vi "gen CE SEM Mask Table.vi"(6 "Mask Type Info":T2, 8 "error in (no error)":errorcluster, 9 "RU Type (0=Full Mask)":i32, 10 "Center Freq":dbl, 11 "SA Measurement in":refnum<class "SA Measurement.lvclass">) -> (0 "error out":errorcluster, 1 "SEM Lower Mask Table":T1(array[cluster]), 2 "SEM Upper Mask Table":T1(array[cluster]), 3 "SA Measurement out":refnum<class "SA Measurement.lvclass">)   [LabVIEW 2023, in "Spectrum Analyzer.lvlib" / "SA Measurement.lvclass"]
uses:
  SA Measurement.lvclass
  SA Measurement.lvclass/SA Measurement.ctl
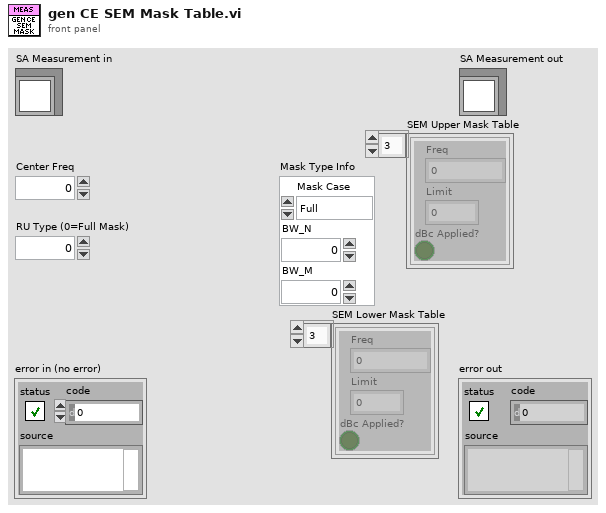
[diagram p1: front panel]
types:
  T1 = cluster{"Freq":dbl, "Limit":dbl, "dBc Applied?":bool}[]
  T2 = cluster{"Mask Case":enum16{"Full", "Case 1", "Case 2", "Case 3", "Case 1+2"}, "BW_N":dbl, "BW_M":dbl}
  T3 = cluster{"Freq":dbl, "Limit":dbl, "dBc Applied?":bool}
  T4 = enum16{"Full", "Case 1", "Case 2", "Case 3", "Case 1+2"}
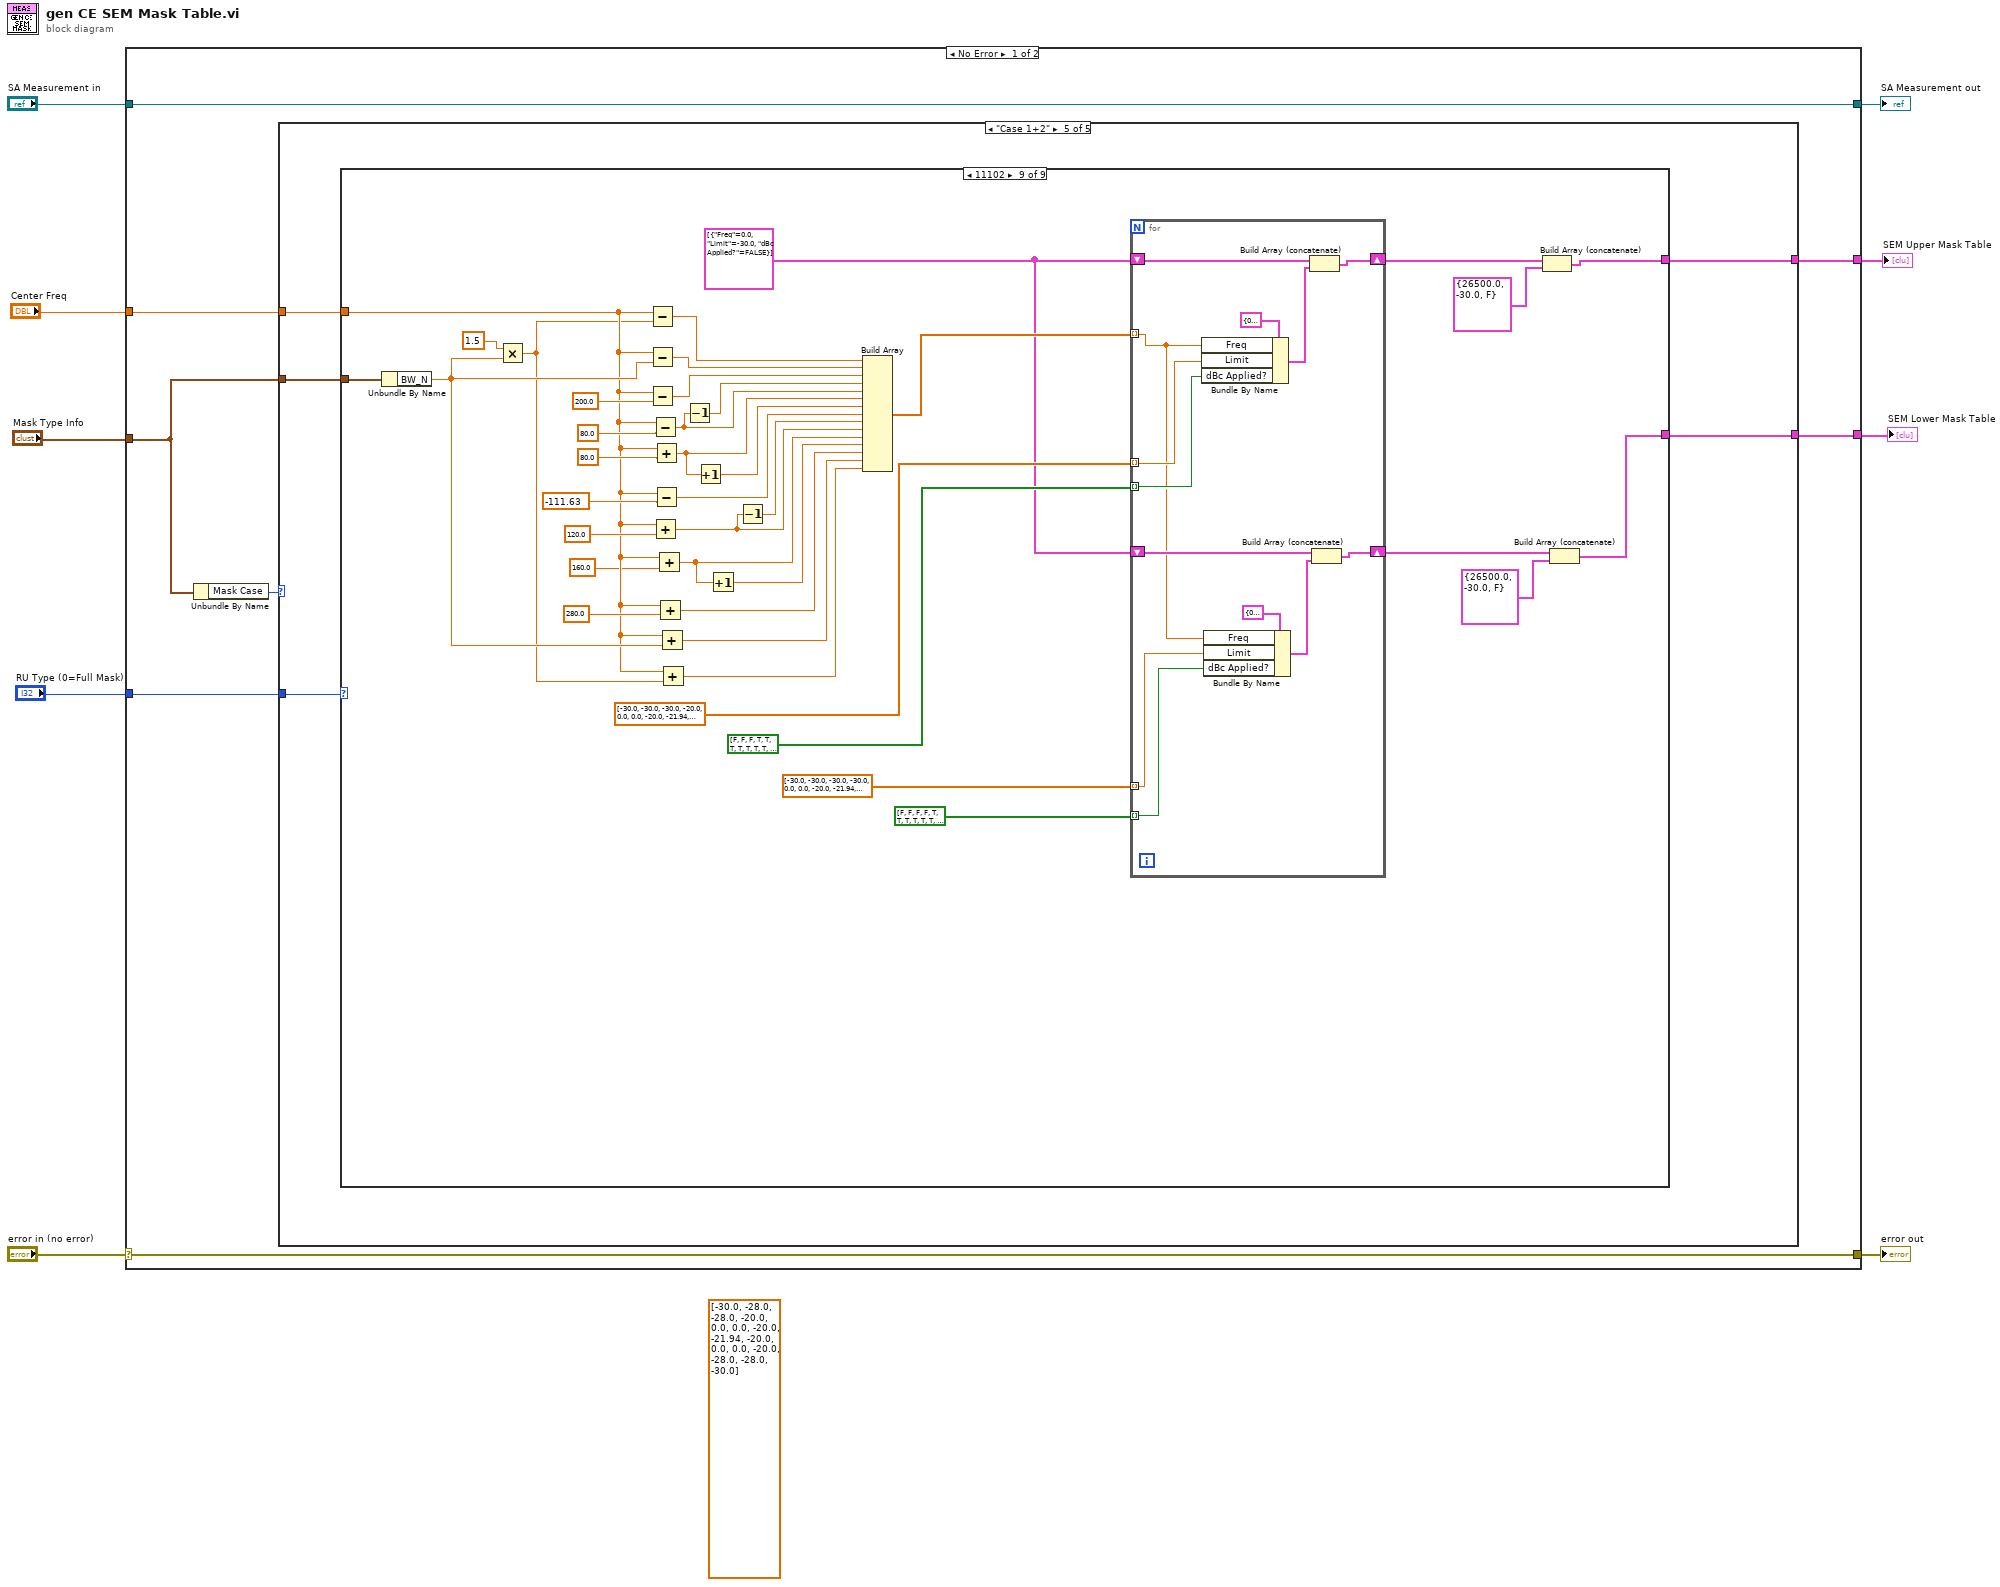
[diagram p0: block diagram]
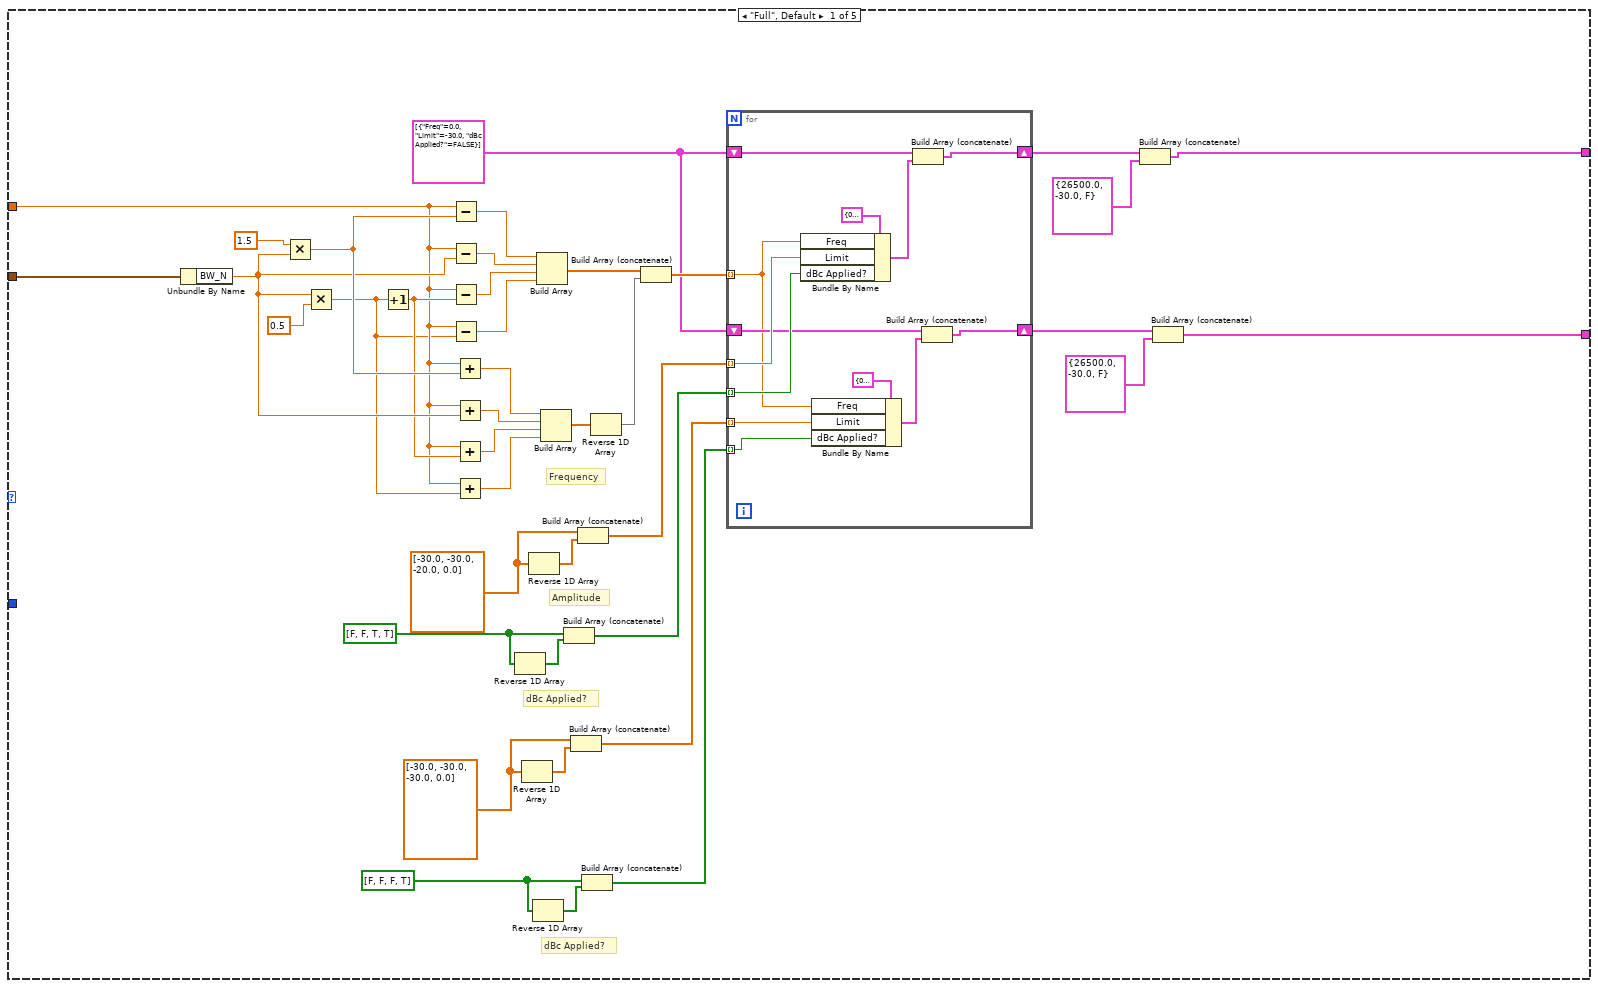
[diagram p2: hidden frame]
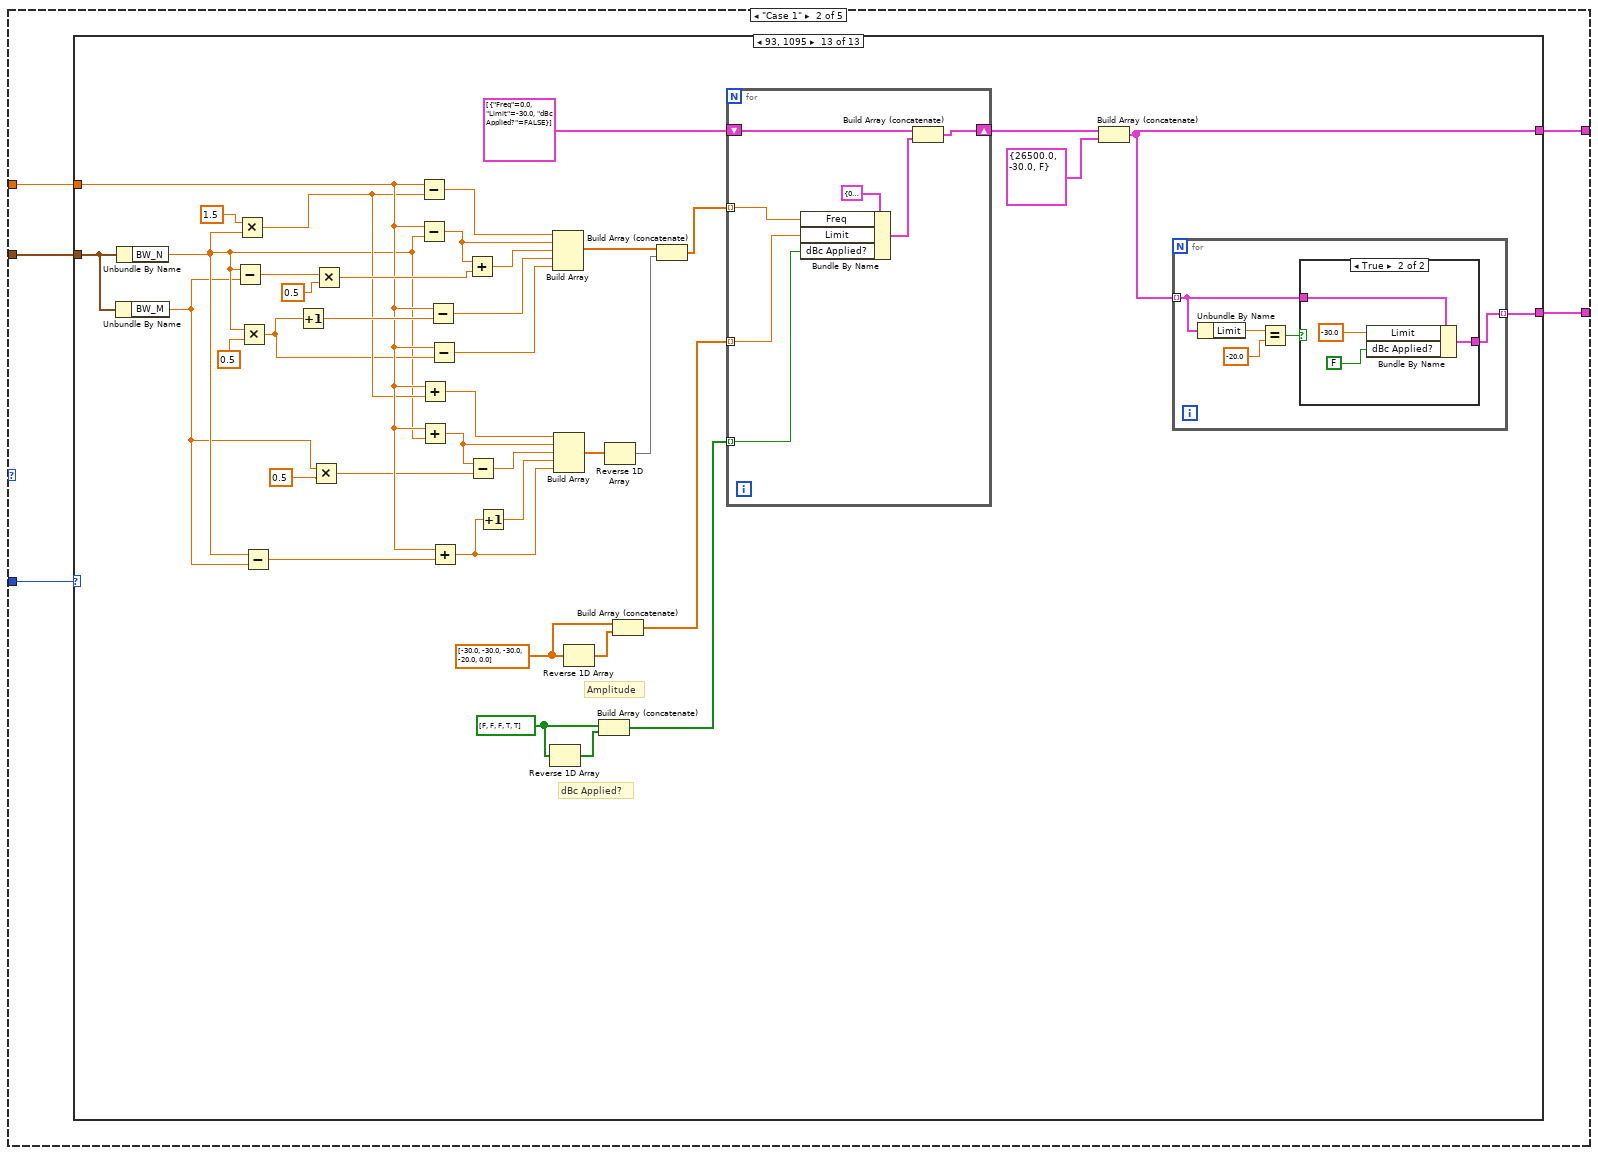
[diagram p3: hidden frame]
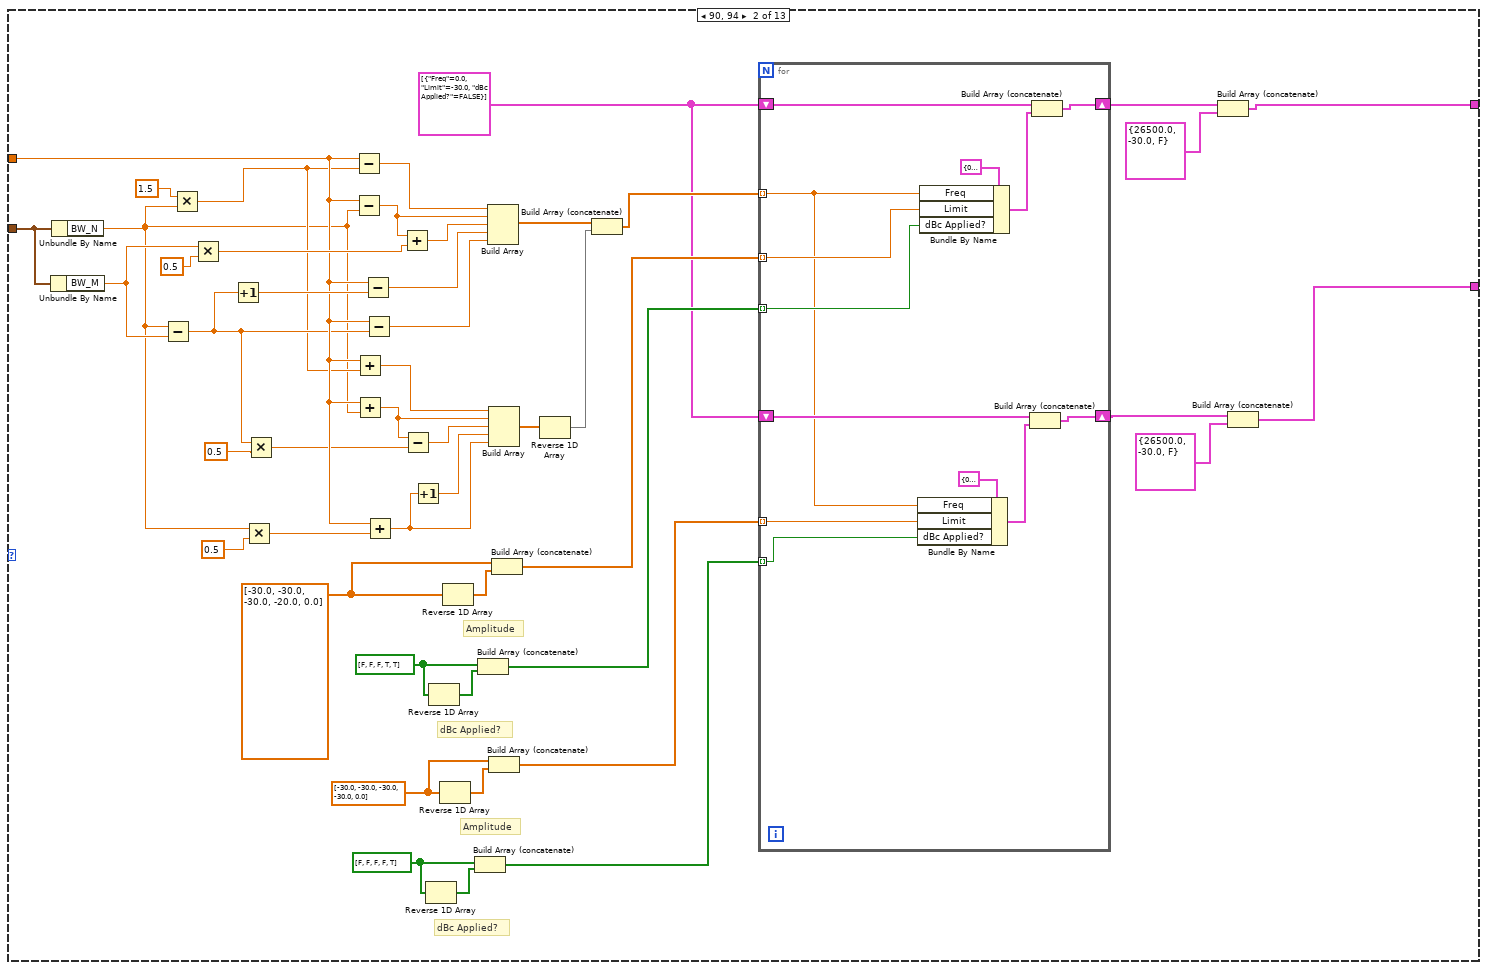
[diagram p5: hidden frame]
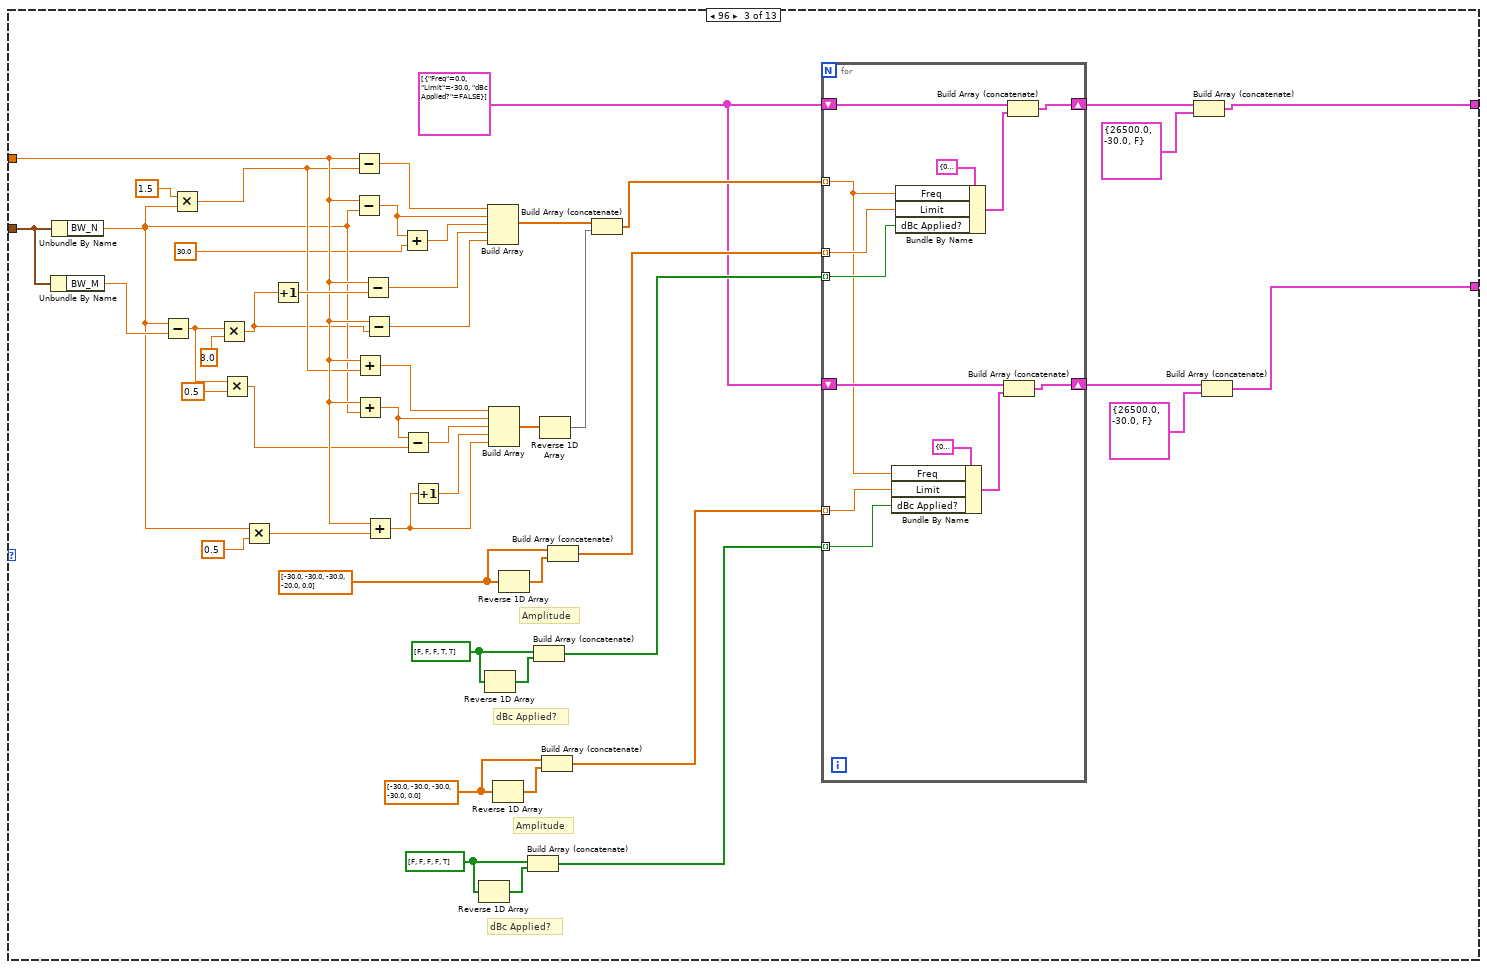
[diagram p6: hidden frame]
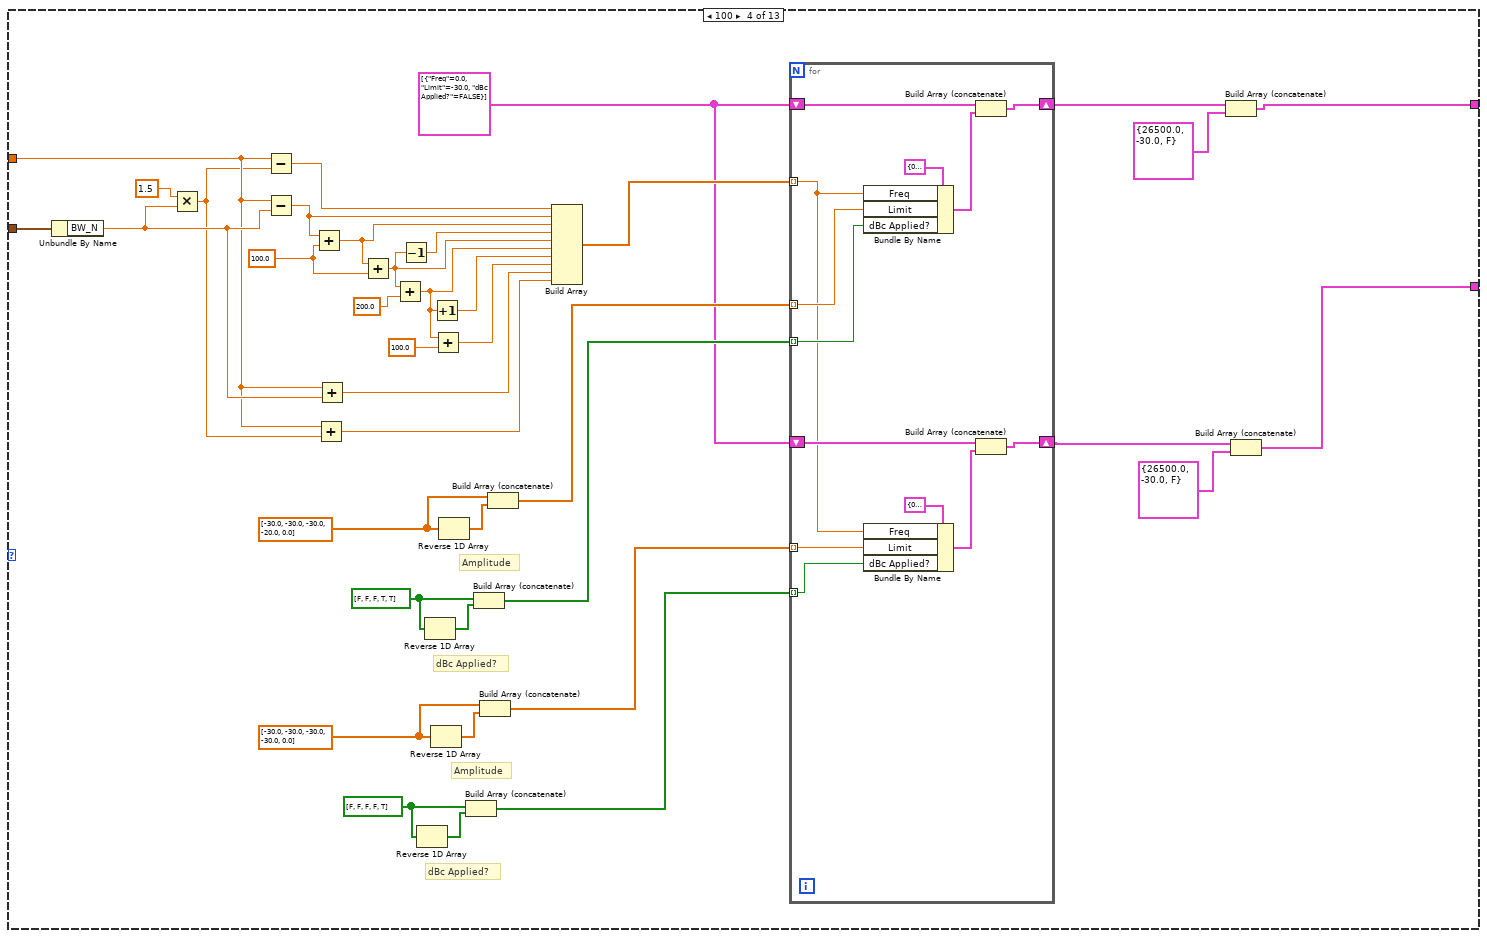
[diagram p7: hidden frame]
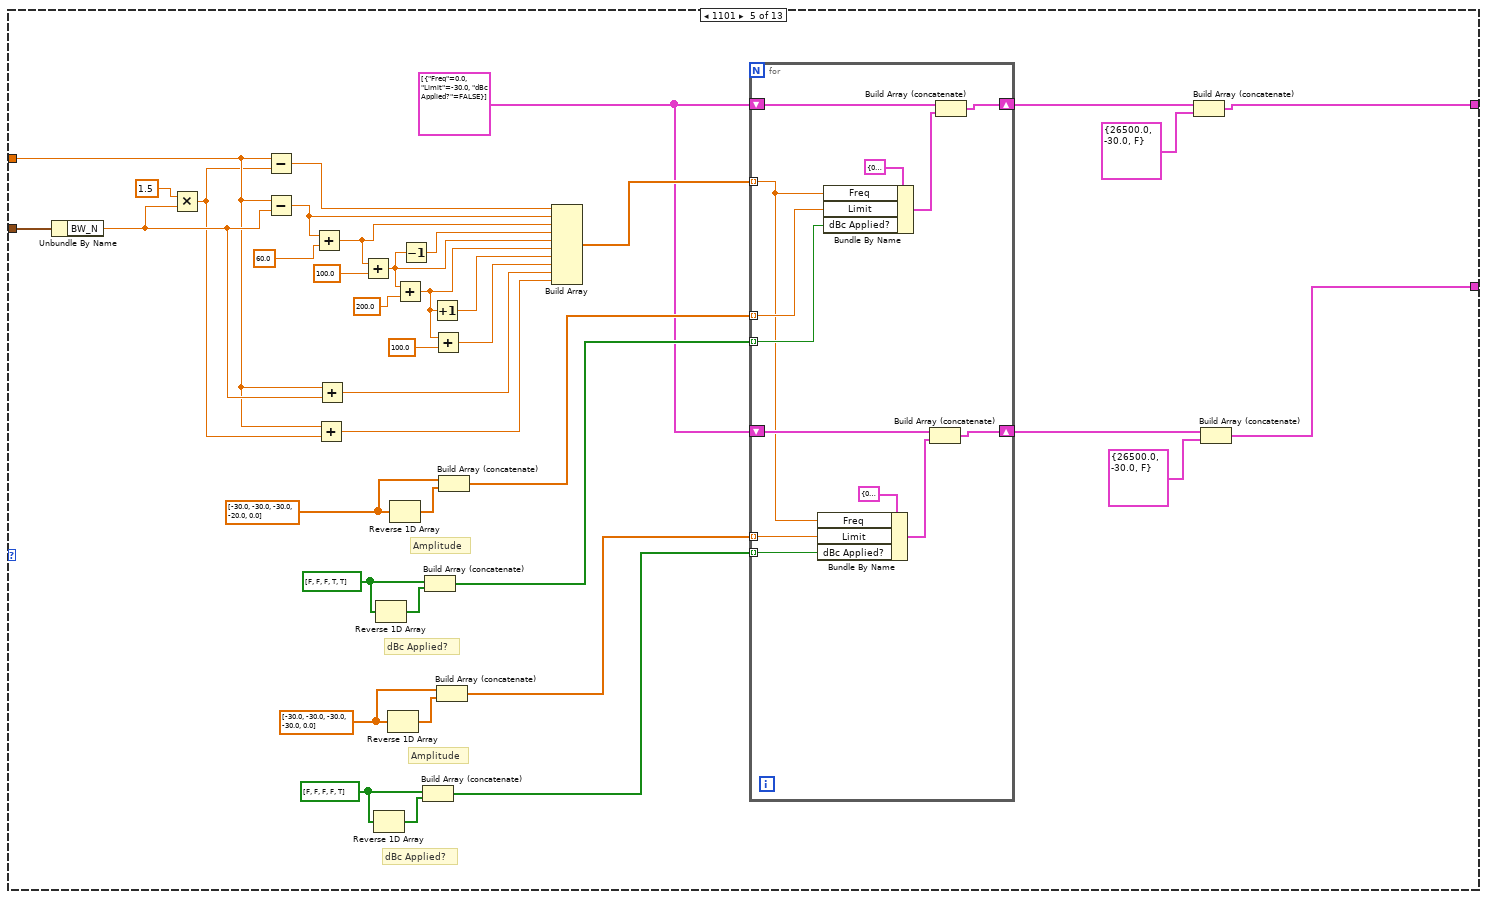
[diagram p8: hidden frame]
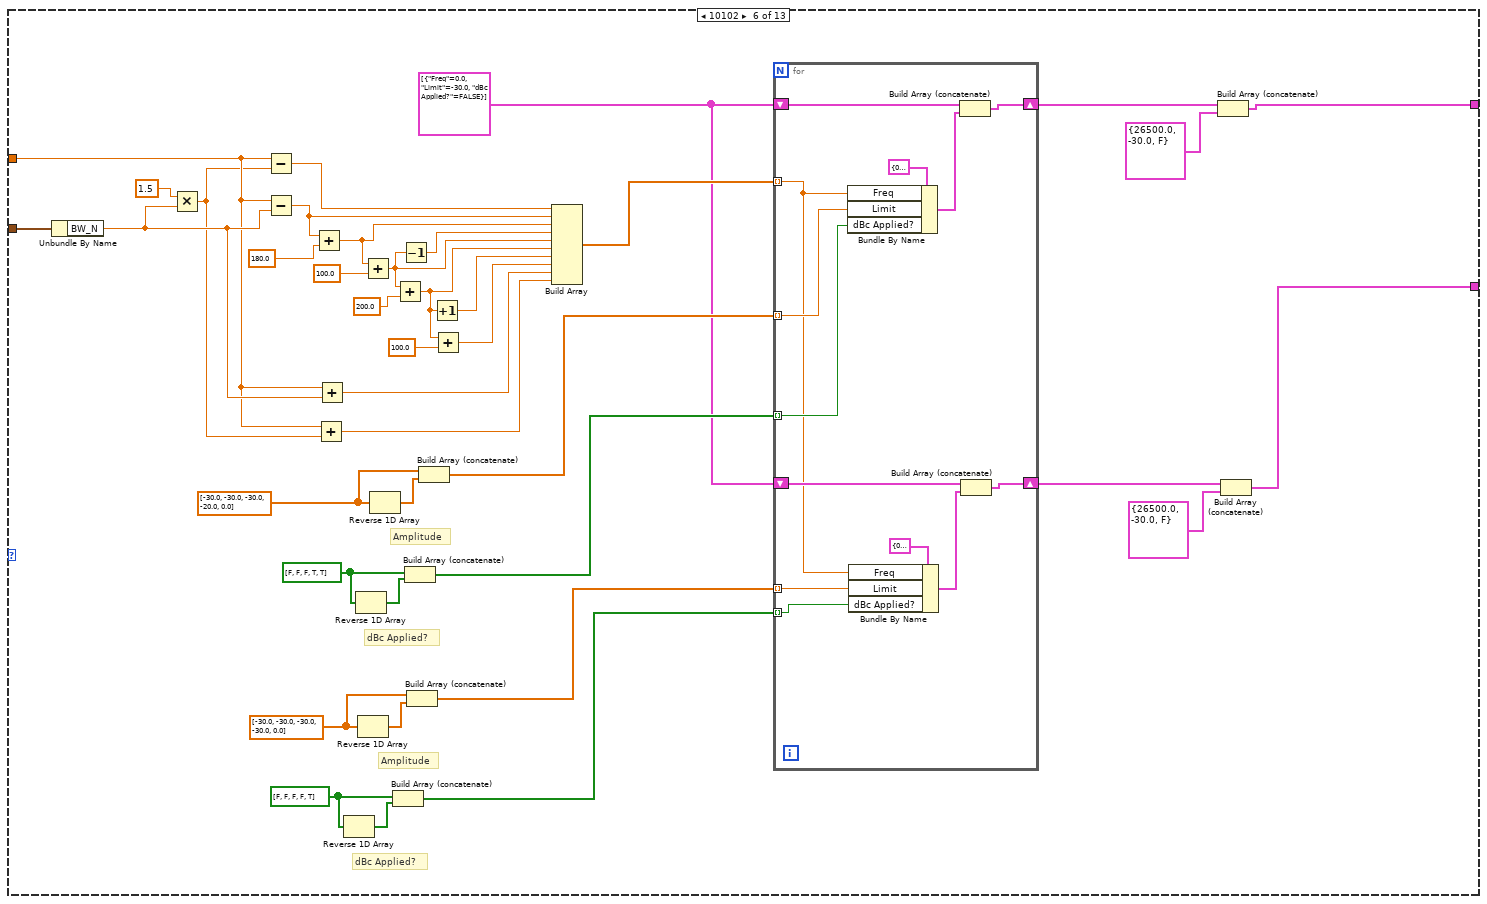
[diagram p9: hidden frame]
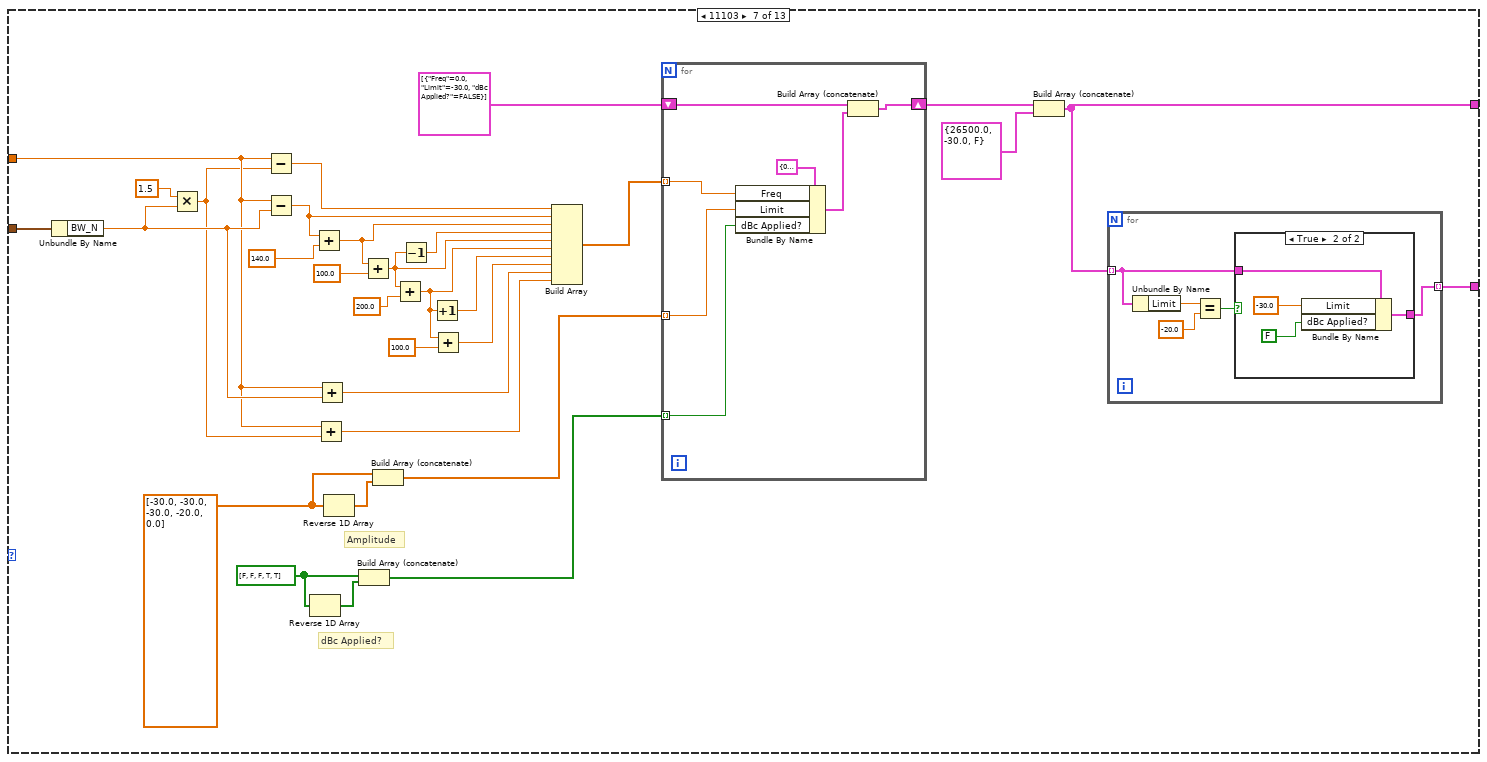
[diagram p10: hidden frame]
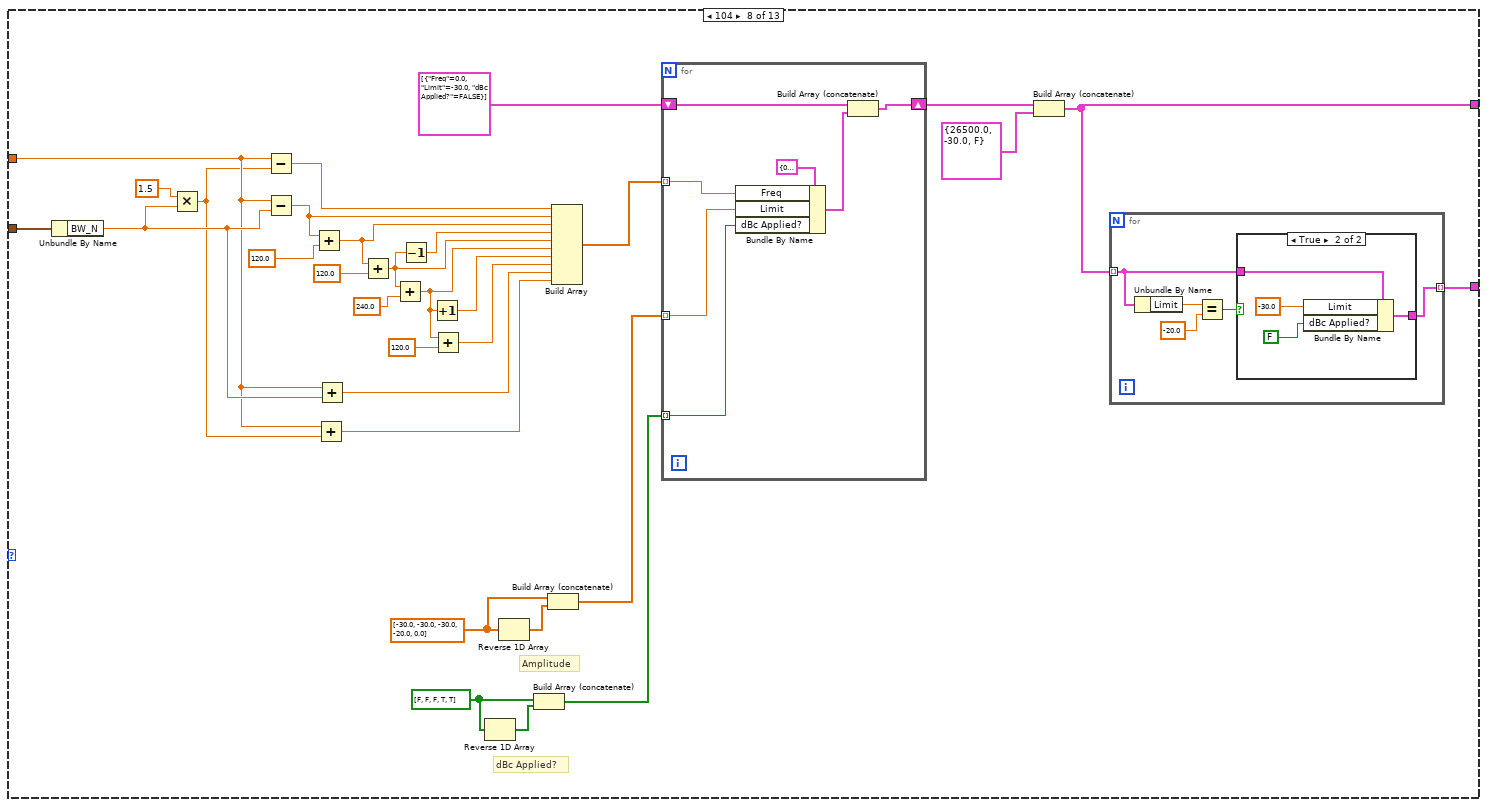
[diagram p12: hidden frame]
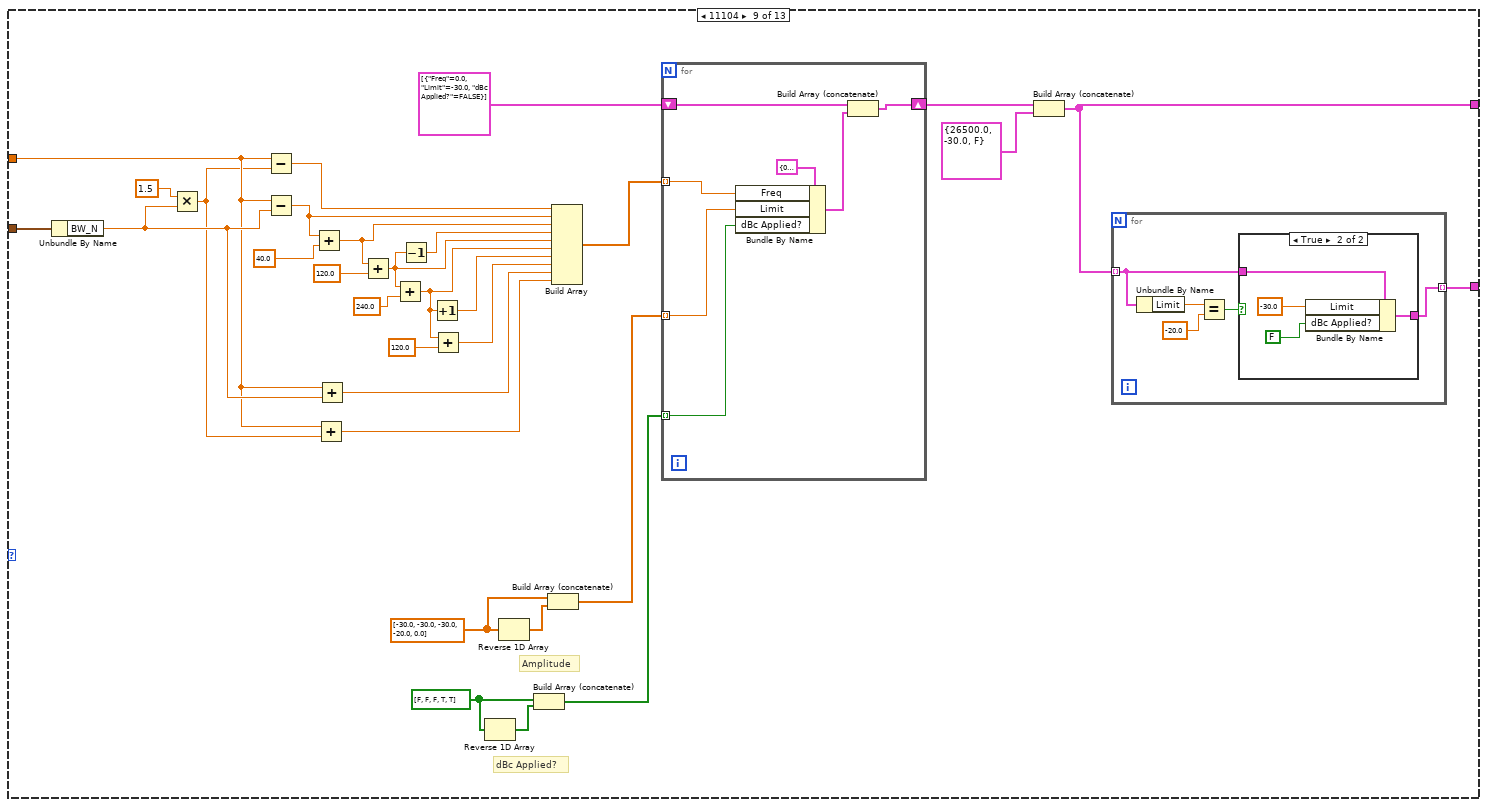
[diagram p14: hidden frame]
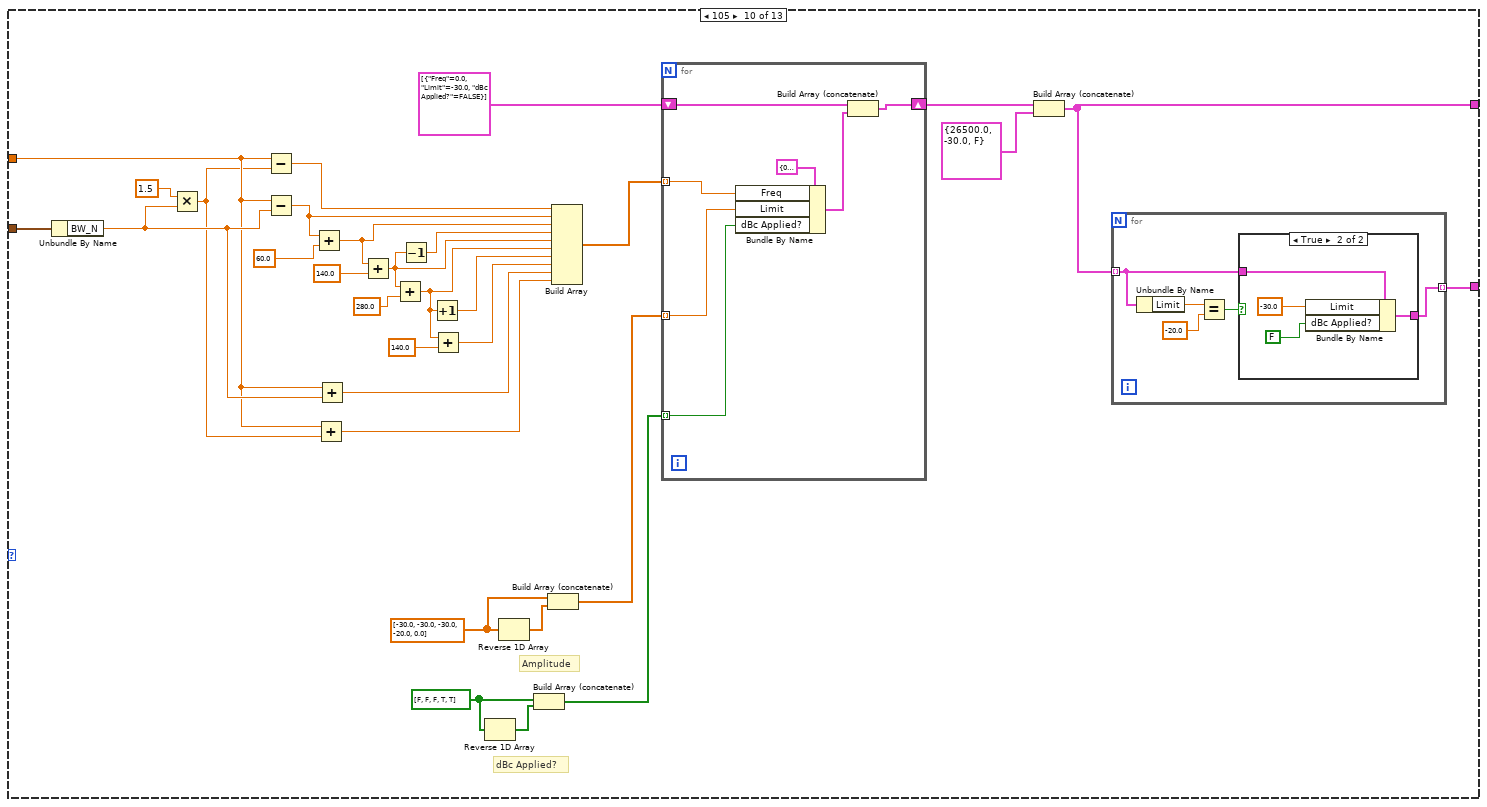
[diagram p16: hidden frame]
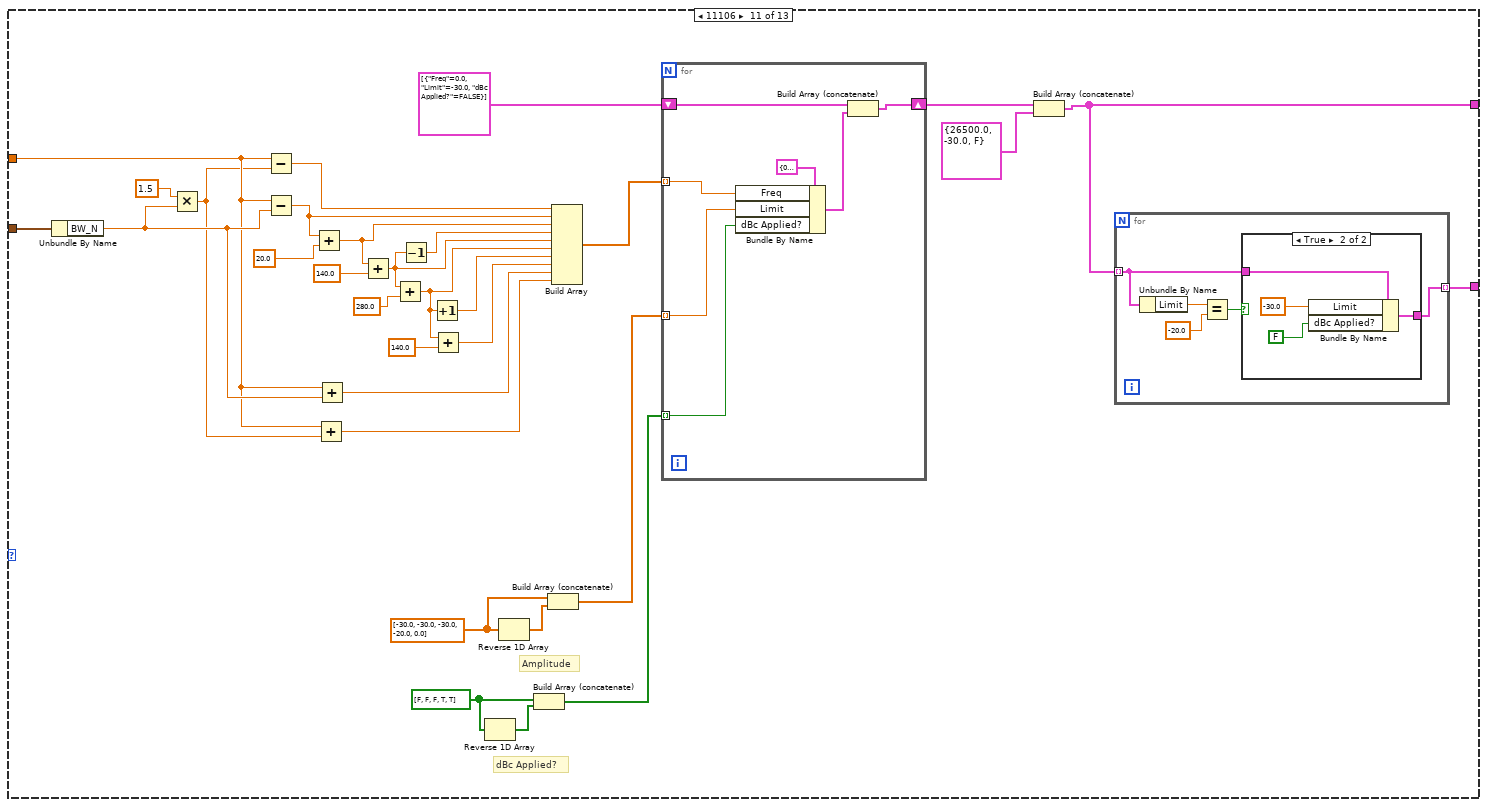
[diagram p18: hidden frame]
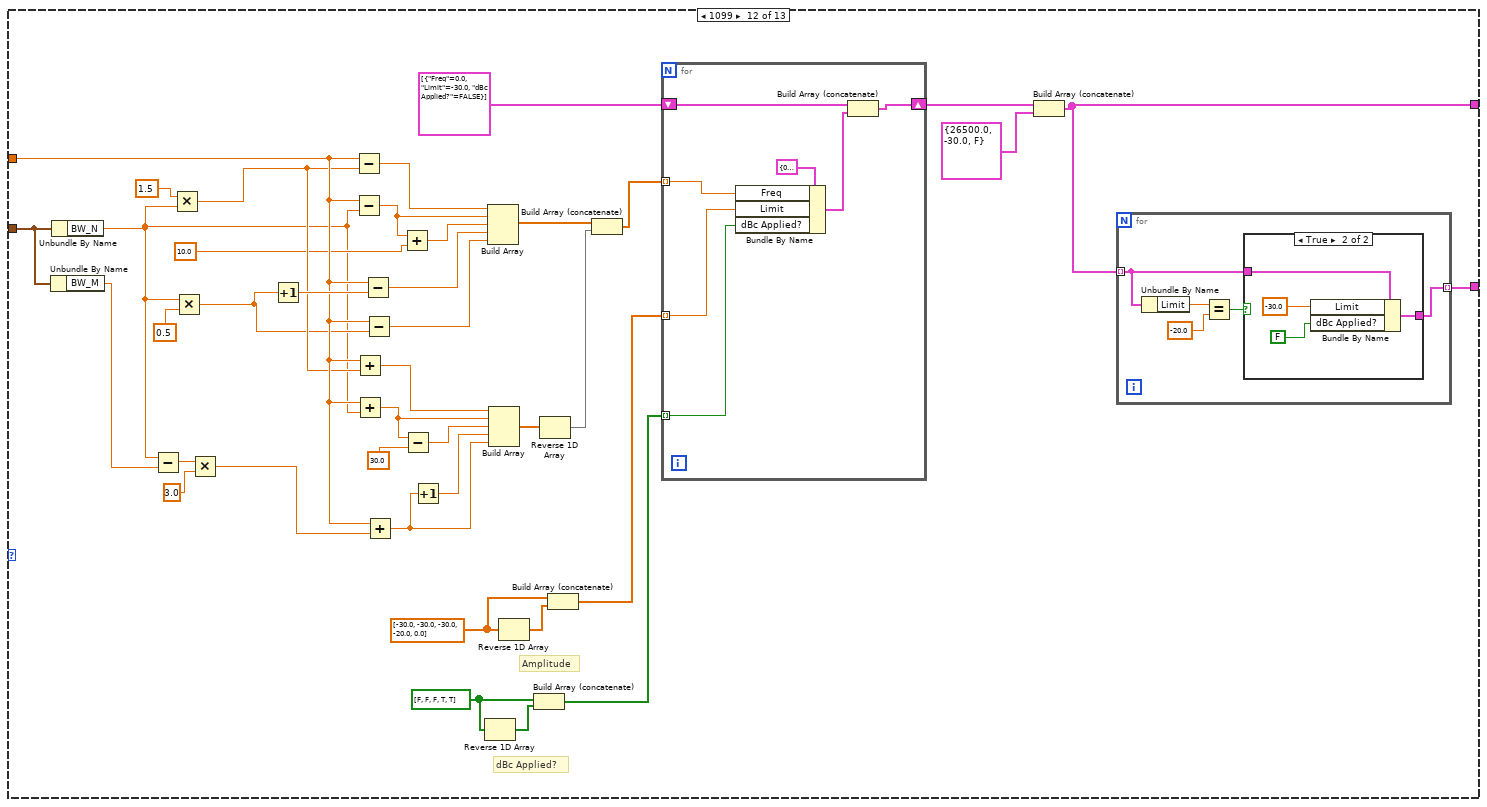
[diagram p20: hidden frame]
diagram:
  (unwired) dbl[] [-30.0, -28.0, -28.0, -20.0, 0.0, 0.0, -20.0, -21.94, -20.0, 0.0, 0.0, -20.0, -28.0, -28.0, -30.0]
  n1 = case shown="No Error" "error in (no error)" {
    selector: "error in (no error)" -> [w16 w2053]
    tunnel: [w16 w2053] -> w8
    tunnel: [w17 w2052] -> w6
    tunnel: "SA Measurement in" -> [w17 w2052]
    tunnel: "Mask Type Info" -> [w13 _]
    tunnel: "Center Freq" -> [w14 _]
    tunnel: "RU Type (0=Full Mask)" -> [w12 _]
    tunnel: [w11 _] -> w2
    tunnel: [w10 _] -> w1
    frame No Error {
      n2 = Unbundle By Name(w13) -> ("Mask Case"=w15:T4)
      n3 = case shown="\"Case 1+2\"" w15 {
        tunnel: w14 -> [w36 w72 w706 w1119 w1634]
        tunnel: w13 -> [w56 w73 w707 w1120 w1635]
        tunnel: [w28 w74 w708 w1121 w1636] -> w11
        tunnel: w12 -> [_ w71 w705 w1118 w1633]
        tunnel: [w24 w70 w704 w1117 w1632] -> w10
        frame "Full", Default {
          w20 = bool[] [FALSE, FALSE, FALSE, TRUE]
          w22 = dbl[] [-30.0, -30.0, -30.0, 0.0]
          w27 = T1 [{"Freq"=0.0, "Limit"=-30.0, "dBc Applied?"=FALSE}] ("value")
          w45 = bool[] [FALSE, FALSE, TRUE, TRUE]
          w49 = dbl[] [-30.0, -30.0, -20.0, 0.0]
          # "dBc Applied?"
          # "dBc Applied?"
          # "Amplitude"
          # "Frequency"
          n4 = Unbundle By Name(w56) -> ("BW_N"=w38:dbl)
          n5 = Multiply(x=1.5, y=w38) -> (x*y=w39:dbl)
          n6 = Multiply(x=w38, y=0.5) -> (x*y=w35:dbl)
          n7 = Increment(x=w35) -> (x+1=w37:dbl)
          n8 = Subtract(x=w36, y=w39) -> (x-y=w53:dbl)
          n9 = Subtract(x=w36, y=w38) -> (x-y=w52:dbl)
          n10 = Subtract(x=w36, y=w37) -> (x-y=w50:dbl)
          n11 = Subtract(x=w36, y=w35) -> (x-y=w51:dbl)
          n12 = Add(x=w36, y=w39) -> (x+y=w40:dbl)
          n13 = Add(x=w36, y=w38) -> (x+y=w41:dbl)
          n14 = Add(x=w36, y=w37) -> (x+y=w43:dbl)
          n15 = Add(x=w36, y=w35) -> (x+y=w42:dbl)
          n16 = Reverse 1D Array(array=w45) -> (reversed array=w46:bool[])
          n17 = Reverse 1D Array(array=w22) -> (reversed array=w23:dbl[])
          n18 = Reverse 1D Array(array=w49) -> (reversed array=w48:dbl[])
          n19 = Reverse 1D Array(array=w20) -> (reversed array=w19:bool[])
          n20 = Build Array(w53, w52, w50, w51) -> (w33:dbl[])
          n21 = Build Array(w40, w41, w43, w42) -> (w34:dbl[])
          n22 = Build Array (concatenate)(w45, w46) -> (w44:bool[])
          n23 = Build Array (concatenate)(w22, w23) -> (w21:dbl[])
          n24 = Build Array (concatenate)(w49, w48) -> (w47:dbl[])
          n25 = Build Array (concatenate)(w20, w19) -> (w18:bool[])
          n26 = Reverse 1D Array(array=w34) -> (reversed array=w32:dbl[])
          n27 = Build Array (concatenate)(w33, w32) -> (w31:dbl[])
          n28 = for {
            tunnel: w31 -> [w59] mode=indexing
            tunnel: w47 -> [w68] mode=indexing
            tunnel: w44 -> [w67] mode=indexing
            shift-right: [w64] -> w30
            shift-left: w27 -> [w66]
            shift-right: [w61] -> w25
            shift-left: w27 -> [w62]
            tunnel: w21 -> [w58] mode=indexing
            tunnel: w18 -> [w57] mode=indexing
            n29 = Bundle By Name(cluster=T3 {"Freq"=0.0, "Limit"=0.0, "dBc Applied?"=FALSE} ("Mask Table"), "Freq"=w59, "Limit"=w68, "dBc Applied?"=w67) -> (w65:T3)
            n30 = Bundle By Name(cluster=T3 {"Freq"=0.0, "Limit"=0.0, "dBc Applied?"=FALSE} ("Mask Table"), "Freq"=w59, "Limit"=w58, "dBc Applied?"=w57) -> (w60:T3)
            n31 = Build Array (concatenate)(w66, w65) -> (w64:T1)
            n32 = Build Array (concatenate)(w62, w60) -> (w61:T1)
          }
          n33 = Build Array (concatenate)(w30, T3 {"Freq"=26500.0, "Limit"=-30.0, "dBc Applied?"=FALSE} ("Mask Table")) -> (w28:T1)
          n34 = Build Array (concatenate)(w25, T3 {"Freq"=26500.0, "Limit"=-30.0, "dBc Applied?"=FALSE} ("Mask Table")) -> (w24:T1)
        }
        frame "Case 1" {
          n35 = case shown="93, 1095" w71 {
            tunnel: [_ w109 w171 w224 w276 w328 w352 w400 w448 w496 w544 w592 w648] -> w74
            tunnel: w73 -> [_ w108 w170 w223 w275 w327 w371 w419 w467 w515 w563 w617 w673]
            tunnel: w72 -> [_ w96 w159 w208 w260 w312 w356 w404 w452 w500 w548 w607 w662]
            tunnel: [_ w75 w135 w196 w247 w299 w351 w399 w447 w495 w543 w591 w647] -> w70
            frame 0, Default {
            }
            frame 90, 94 {
              w84 = dbl[] [-30.0, -30.0, -30.0, -30.0, 0.0]
              w83 = bool[] [FALSE, FALSE, FALSE, FALSE, TRUE]
              w106 = dbl[] [-30.0, -30.0, -30.0, -20.0, 0.0]
              w80 = T1 [{"Freq"=0.0, "Limit"=-30.0, "dBc Applied?"=FALSE}] ("value")
              w115 = bool[] [FALSE, FALSE, FALSE, TRUE, TRUE]
              # "dBc Applied?"
              # "Amplitude"
              # "dBc Applied?"
              # "Amplitude"
              n36 = Unbundle By Name(w108) -> ("BW_M"=w103:dbl)
              n37 = Unbundle By Name(w108) -> ("BW_N"=w91:dbl)
              n38 = Subtract(x=w91, y=w103) -> (x-y=w95:dbl)
              n39 = Multiply(x=1.5, y=w91) -> (x*y=w92:dbl)
              n40 = Multiply(x=w103, y=0.5) -> (x*y=w104:dbl)
              n41 = Increment(x=w95) -> (x+1=w102:dbl)
              n42 = Multiply(x=w91, y=0.5) -> (x*y=w89:dbl)
              n43 = Multiply(x=w95, y=0.5) -> (x*y=w93:dbl)
              n44 = Subtract(x=w96, y=w92) -> (x-y=w119:dbl)
              n45 = Subtract(x=w96, y=w91) -> (x-y=w105:dbl)
              n46 = Add(x=w96, y=w92) -> (x+y=w97:dbl)
              n47 = Add(x=w96, y=w91) -> (x+y=w99:dbl)
              n48 = Subtract(x=w96, y=w102) -> (x-y=w101:dbl)
              n49 = Subtract(x=w96, y=w95) -> (x-y=w100:dbl)
              n50 = Add(x=w96, y=w89) -> (x+y=w88:dbl)
              n51 = Add(x=w105, y=w104) -> (x+y=w107:dbl)
              n52 = Subtract(x=w99, y=w93) -> (x-y=w98:dbl)
              n53 = Increment(x=w88) -> (x+1=w87:dbl)
              n54 = Reverse 1D Array(array=w83) -> (reversed array=w82:bool[])
              n55 = Reverse 1D Array(array=w115) -> (reversed array=w116:bool[])
              n56 = Reverse 1D Array(array=w84) -> (reversed array=w81:dbl[])
              n57 = Reverse 1D Array(array=w106) -> (reversed array=w118:dbl[])
              n58 = Build Array (concatenate)(w83, w82) -> (w78:bool[])
              n59 = Build Array (concatenate)(w115, w116) -> (w114:bool[])
              n60 = Build Array(w119, w105, w107, w101, w100) -> (w113:dbl[])
              n61 = Build Array(w97, w99, w98, w87, w88) -> (w86:dbl[])
              n62 = Build Array (concatenate)(w84, w81) -> (w79:dbl[])
              n63 = Build Array (concatenate)(w106, w118) -> (w117:dbl[])
              n64 = Reverse 1D Array(array=w86) -> (reversed array=w85:dbl[])
              n65 = Build Array (concatenate)(w113, w85) -> (w112:dbl[])
              n66 = for {
                tunnel: w112 -> [w124] mode=indexing
                tunnel: w117 -> [w133] mode=indexing
                tunnel: w114 -> [w132] mode=indexing
                shift-right: [w129] -> w111
                shift-left: w80 -> [w131]
                shift-right: [w125] -> w76
                shift-left: w80 -> [w126]
                tunnel: w79 -> [w123] mode=indexing
                tunnel: w78 -> [w122] mode=indexing
                n67 = Bundle By Name(cluster=T3 {"Freq"=0.0, "Limit"=0.0, "dBc Applied?"=FALSE} ("Mask Table"), "Freq"=w124, "Limit"=w123, "dBc Applied?"=w122) -> (w128:T3)
                n68 = Bundle By Name(cluster=T3 {"Freq"=0.0, "Limit"=0.0, "dBc Applied?"=FALSE} ("Mask Table"), "Freq"=w124, "Limit"=w133, "dBc Applied?"=w132) -> (w130:T3)
                n69 = Build Array (concatenate)(w126, w128) -> (w125:T1)
                n70 = Build Array (concatenate)(w131, w130) -> (w129:T1)
              }
              n71 = Build Array (concatenate)(w111, T3 {"Freq"=26500.0, "Limit"=-30.0, "dBc Applied?"=FALSE} ("Mask Table")) -> (w109:T1)
              n72 = Build Array (concatenate)(w76, T3 {"Freq"=26500.0, "Limit"=-30.0, "dBc Applied?"=FALSE} ("Mask Table")) -> (w75:T1)
            }
            frame 96 {
              w144 = dbl[] [-30.0, -30.0, -30.0, -30.0, 0.0]
              w143 = bool[] [FALSE, FALSE, FALSE, FALSE, TRUE]
              w168 = dbl[] [-30.0, -30.0, -30.0, -20.0, 0.0]
              w139 = T1 [{"Freq"=0.0, "Limit"=-30.0, "dBc Applied?"=FALSE}] ("value")
              w177 = bool[] [FALSE, FALSE, FALSE, TRUE, TRUE]
              # "dBc Applied?"
              # "Amplitude"
              # "dBc Applied?"
              # "Amplitude"
              n73 = Unbundle By Name(w170) -> ("BW_M"=w166:dbl)
              n74 = Unbundle By Name(w170) -> ("BW_N"=w157:dbl)
              n75 = Subtract(x=w157, y=w166) -> (x-y=w148:dbl)
              n76 = Multiply(x=1.5, y=w157) -> (x*y=w158:dbl)
              n77 = Multiply(x=w148, y=3.0) -> (x*y=w146:dbl)
              n78 = Multiply(x=w148, y=0.5) -> (x*y=w145:dbl)
              n79 = Multiply(x=w157, y=0.5) -> (x*y=w155:dbl)
              n80 = Increment(x=w146) -> (x+1=w165:dbl)
              n81 = Subtract(x=w159, y=w158) -> (x-y=w181:dbl)
              n82 = Subtract(x=w159, y=w157) -> (x-y=w167:dbl)
              n83 = Add(x=w159, y=w158) -> (x+y=w160:dbl)
              n84 = Add(x=w159, y=w157) -> (x+y=w162:dbl)
              n85 = Subtract(x=w159, y=w165) -> (x-y=w164:dbl)
              n86 = Subtract(x=w159, y=w146) -> (x-y=w163:dbl)
              n87 = Add(x=w159, y=w155) -> (x+y=w154:dbl)
              n88 = Add(x=w167, y=30.0 ("x")) -> (x+y=w169:dbl)
              n89 = Subtract(x=w162, y=w145) -> (x-y=w161:dbl)
              n90 = Increment(x=w154) -> (x+1=w153:dbl)
              n91 = Reverse 1D Array(array=w143) -> (reversed array=w142:bool[])
              n92 = Reverse 1D Array(array=w177) -> (reversed array=w178:bool[])
              n93 = Build Array(w181, w167, w169, w164, w163) -> (w175:dbl[])
              n94 = Build Array(w160, w162, w161, w153, w154) -> (w152:dbl[])
              n95 = Reverse 1D Array(array=w144) -> (reversed array=w141:dbl[])
              n96 = Reverse 1D Array(array=w168) -> (reversed array=w180:dbl[])
              n97 = Build Array (concatenate)(w143, w142) -> (w138:bool[])
              n98 = Build Array (concatenate)(w177, w178) -> (w176:bool[])
              n99 = Reverse 1D Array(array=w152) -> (reversed array=w151:dbl[])
              n100 = Build Array (concatenate)(w144, w141) -> (w140:dbl[])
              n101 = Build Array (concatenate)(w168, w180) -> (w179:dbl[])
              n102 = Build Array (concatenate)(w175, w151) -> (w174:dbl[])
              n103 = for {
                tunnel: w174 -> [w185] mode=indexing
                tunnel: w179 -> [w194] mode=indexing
                tunnel: w176 -> [w193] mode=indexing
                shift-right: [w190] -> w173
                shift-left: w139 -> [w192]
                tunnel: w140 -> [w184] mode=indexing
                shift-right: [w186] -> w136
                shift-left: w139 -> [w187]
                tunnel: w138 -> [w183] mode=indexing
                n104 = Bundle By Name(cluster=T3 {"Freq"=0.0, "Limit"=0.0, "dBc Applied?"=FALSE} ("Mask Table"), "Freq"=w185, "Limit"=w184, "dBc Applied?"=w183) -> (w189:T3)
                n105 = Bundle By Name(cluster=T3 {"Freq"=0.0, "Limit"=0.0, "dBc Applied?"=FALSE} ("Mask Table"), "Freq"=w185, "Limit"=w194, "dBc Applied?"=w193) -> (w191:T3)
                n106 = Build Array (concatenate)(w187, w189) -> (w186:T1)
                n107 = Build Array (concatenate)(w192, w191) -> (w190:T1)
              }
              n108 = Build Array (concatenate)(w173, T3 {"Freq"=26500.0, "Limit"=-30.0, "dBc Applied?"=FALSE} ("Mask Table")) -> (w171:T1)
              n109 = Build Array (concatenate)(w136, T3 {"Freq"=26500.0, "Limit"=-30.0, "dBc Applied?"=FALSE} ("Mask Table")) -> (w135:T1)
            }
            frame 100 {
              w204 = dbl[] [-30.0, -30.0, -30.0, -30.0, 0.0]
              w203 = bool[] [FALSE, FALSE, FALSE, FALSE, TRUE]
              w219 = 100.0 ("x")
              w222 = dbl[] [-30.0, -30.0, -30.0, -20.0, 0.0]
              w205 = T1 [{"Freq"=0.0, "Limit"=-30.0, "dBc Applied?"=FALSE}] ("value")
              w228 = bool[] [FALSE, FALSE, FALSE, TRUE, TRUE]
              # "dBc Applied?"
              # "Amplitude"
              # "dBc Applied?"
              # "Amplitude"
              n110 = Unbundle By Name(w223) -> ("BW_N"=w210:dbl)
              n111 = Multiply(x=1.5, y=w210) -> (x*y=w207:dbl)
              n112 = Subtract(x=w208, y=w207) -> (x-y=w232:dbl)
              n113 = Subtract(x=w208, y=w210) -> (x-y=w221:dbl)
              n114 = Add(x=w221, y=w219) -> (x+y=w220:dbl)
              n115 = Add(x=w208, y=w207) -> (x+y=w206:dbl)
              n116 = Add(x=w208, y=w210) -> (x+y=w209:dbl)
              n117 = Add(x=w220, y=w219) -> (x+y=w216:dbl)
              n118 = Add(x=w216, y=200.0) -> (x+y=w213:dbl)
              n119 = Decrement(x=w216) -> (x-1=w218:dbl)
              n120 = Reverse 1D Array(array=w203) -> (reversed array=w202:bool[])
              n121 = Reverse 1D Array(array=w228) -> (reversed array=w229:bool[])
              n122 = Reverse 1D Array(array=w204) -> (reversed array=w201:dbl[])
              n123 = Increment(x=w213) -> (x+1=w214:dbl)
              n124 = Add(x=w213, y=100.0) -> (x+y=w211:dbl)
              n125 = Reverse 1D Array(array=w222) -> (reversed array=w231:dbl[])
              n126 = Build Array (concatenate)(w203, w202) -> (w199:bool[])
              n127 = Build Array (concatenate)(w228, w229) -> (w227:bool[])
              n128 = Build Array (concatenate)(w204, w201) -> (w200:dbl[])
              n129 = Build Array (concatenate)(w222, w231) -> (w230:dbl[])
              n130 = Build Array(w232, w221, w220, w218, w216, w213, w214, w211, w209, w206) -> (w217:dbl[])
              n131 = for {
                tunnel: w217 -> [w236] mode=indexing
                tunnel: w230 -> [w245] mode=indexing
                tunnel: w227 -> [w244] mode=indexing
                shift-right: [w241] -> w226
                shift-left: w205 -> [w243]
                shift-right: [w237] -> w197
                shift-left: w205 -> [w238]
                tunnel: w200 -> [w235] mode=indexing
                tunnel: w199 -> [w234] mode=indexing
                n132 = Bundle By Name(cluster=T3 {"Freq"=0.0, "Limit"=0.0, "dBc Applied?"=FALSE} ("Mask Table"), "Freq"=w236, "Limit"=w245, "dBc Applied?"=w244) -> (w242:T3)
                n133 = Bundle By Name(cluster=T3 {"Freq"=0.0, "Limit"=0.0, "dBc Applied?"=FALSE} ("Mask Table"), "Freq"=w236, "Limit"=w235, "dBc Applied?"=w234) -> (w240:T3)
                n134 = Build Array (concatenate)(w243, w242) -> (w241:T1)
                n135 = Build Array (concatenate)(w238, w240) -> (w237:T1)
              }
              n136 = Build Array (concatenate)(w226, T3 {"Freq"=26500.0, "Limit"=-30.0, "dBc Applied?"=FALSE} ("Mask Table")) -> (w224:T1)
              n137 = Build Array (concatenate)(w197, T3 {"Freq"=26500.0, "Limit"=-30.0, "dBc Applied?"=FALSE} ("Mask Table")) -> (w196:T1)
            }
            frame 1101 {
              w255 = dbl[] [-30.0, -30.0, -30.0, -30.0, 0.0]
              w254 = bool[] [FALSE, FALSE, FALSE, FALSE, TRUE]
              w274 = dbl[] [-30.0, -30.0, -30.0, -20.0, 0.0]
              w256 = T1 [{"Freq"=0.0, "Limit"=-30.0, "dBc Applied?"=FALSE}] ("value")
              w280 = bool[] [FALSE, FALSE, FALSE, TRUE, TRUE]
              # "dBc Applied?"
              # "Amplitude"
              # "dBc Applied?"
              # "Amplitude"
              n138 = Unbundle By Name(w275) -> ("BW_N"=w262:dbl)
              n139 = Multiply(x=1.5, y=w262) -> (x*y=w259:dbl)
              n140 = Subtract(x=w260, y=w259) -> (x-y=w284:dbl)
              n141 = Subtract(x=w260, y=w262) -> (x-y=w273:dbl)
              n142 = Add(x=w273, y=60.0 ("x")) -> (x+y=w272:dbl)
              n143 = Add(x=w260, y=w259) -> (x+y=w258:dbl)
              n144 = Add(x=w260, y=w262) -> (x+y=w261:dbl)
              n145 = Add(x=w272, y=100.0) -> (x+y=w268:dbl)
              n146 = Reverse 1D Array(array=w254) -> (reversed array=w253:bool[])
              n147 = Reverse 1D Array(array=w280) -> (reversed array=w281:bool[])
              n148 = Reverse 1D Array(array=w255) -> (reversed array=w252:dbl[])
              n149 = Reverse 1D Array(array=w274) -> (reversed array=w283:dbl[])
              n150 = Add(x=w268, y=200.0) -> (x+y=w265:dbl)
              n151 = Decrement(x=w268) -> (x-1=w270:dbl)
              n152 = Build Array (concatenate)(w254, w253) -> (w250:bool[])
              n153 = Build Array (concatenate)(w280, w281) -> (w279:bool[])
              n154 = Increment(x=w265) -> (x+1=w266:dbl)
              n155 = Add(x=w265, y=100.0) -> (x+y=w263:dbl)
              n156 = Build Array (concatenate)(w255, w252) -> (w251:dbl[])
              n157 = Build Array (concatenate)(w274, w283) -> (w282:dbl[])
              n158 = Build Array(w284, w273, w272, w270, w268, w265, w266, w263, w261, w258) -> (w269:dbl[])
              n159 = for {
                tunnel: w269 -> [w288] mode=indexing
                tunnel: w282 -> [w297] mode=indexing
                tunnel: w279 -> [w296] mode=indexing
                shift-right: [w293] -> w278
                shift-left: w256 -> [w295]
                shift-right: [w289] -> w248
                shift-left: w256 -> [w290]
                tunnel: w251 -> [w287] mode=indexing
                tunnel: w250 -> [w286] mode=indexing
                n160 = Bundle By Name(cluster=T3 {"Freq"=0.0, "Limit"=0.0, "dBc Applied?"=FALSE} ("Mask Table"), "Freq"=w288, "Limit"=w287, "dBc Applied?"=w286) -> (w292:T3)
                n161 = Bundle By Name(cluster=T3 {"Freq"=0.0, "Limit"=0.0, "dBc Applied?"=FALSE} ("Mask Table"), "Freq"=w288, "Limit"=w297, "dBc Applied?"=w296) -> (w294:T3)
                n162 = Build Array (concatenate)(w290, w292) -> (w289:T1)
                n163 = Build Array (concatenate)(w295, w294) -> (w293:T1)
              }
              n164 = Build Array (concatenate)(w278, T3 {"Freq"=26500.0, "Limit"=-30.0, "dBc Applied?"=FALSE} ("Mask Table")) -> (w276:T1)
              n165 = Build Array (concatenate)(w248, T3 {"Freq"=26500.0, "Limit"=-30.0, "dBc Applied?"=FALSE} ("Mask Table")) -> (w247:T1)
            }
            frame 10102 {
              w307 = dbl[] [-30.0, -30.0, -30.0, -30.0, 0.0]
              w306 = bool[] [FALSE, FALSE, FALSE, FALSE, TRUE]
              w326 = dbl[] [-30.0, -30.0, -30.0, -20.0, 0.0]
              w308 = T1 [{"Freq"=0.0, "Limit"=-30.0, "dBc Applied?"=FALSE}] ("value")
              w332 = bool[] [FALSE, FALSE, FALSE, TRUE, TRUE]
              # "dBc Applied?"
              # "Amplitude"
              # "dBc Applied?"
              # "Amplitude"
              n166 = Unbundle By Name(w327) -> ("BW_N"=w314:dbl)
              n167 = Multiply(x=1.5, y=w314) -> (x*y=w311:dbl)
              n168 = Subtract(x=w312, y=w311) -> (x-y=w336:dbl)
              n169 = Subtract(x=w312, y=w314) -> (x-y=w325:dbl)
              n170 = Add(x=w325, y=180.0 ("x")) -> (x+y=w324:dbl)
              n171 = Add(x=w312, y=w311) -> (x+y=w310:dbl)
              n172 = Add(x=w312, y=w314) -> (x+y=w313:dbl)
              n173 = Reverse 1D Array(array=w306) -> (reversed array=w305:bool[])
              n174 = Reverse 1D Array(array=w332) -> (reversed array=w333:bool[])
              n175 = Reverse 1D Array(array=w307) -> (reversed array=w304:dbl[])
              n176 = Add(x=w324, y=100.0) -> (x+y=w320:dbl)
              n177 = Reverse 1D Array(array=w326) -> (reversed array=w335:dbl[])
              n178 = Build Array (concatenate)(w306, w305) -> (w302:bool[])
              n179 = Add(x=w320, y=200.0) -> (x+y=w317:dbl)
              n180 = Decrement(x=w320) -> (x-1=w322:dbl)
              n181 = Build Array (concatenate)(w332, w333) -> (w331:bool[])
              n182 = Build Array (concatenate)(w307, w304) -> (w303:dbl[])
              n183 = Build Array (concatenate)(w326, w335) -> (w334:dbl[])
              n184 = Increment(x=w317) -> (x+1=w318:dbl)
              n185 = Add(x=w317, y=100.0) -> (x+y=w315:dbl)
              n186 = Build Array(w336, w325, w324, w322, w320, w317, w318, w315, w313, w310) -> (w321:dbl[])
              n187 = for {
                tunnel: w321 -> [w340] mode=indexing
                tunnel: w334 -> [w349] mode=indexing
                tunnel: w331 -> [w348] mode=indexing
                shift-right: [w345] -> w330
                shift-left: w308 -> [w347]
                shift-right: [w341] -> w300
                shift-left: w308 -> [w342]
                tunnel: w303 -> [w339] mode=indexing
                tunnel: w302 -> [w338] mode=indexing
                n188 = Bundle By Name(cluster=T3 {"Freq"=0.0, "Limit"=0.0, "dBc Applied?"=FALSE} ("Mask Table"), "Freq"=w340, "Limit"=w349, "dBc Applied?"=w348) -> (w346:T3)
                n189 = Bundle By Name(cluster=T3 {"Freq"=0.0, "Limit"=0.0, "dBc Applied?"=FALSE} ("Mask Table"), "Freq"=w340, "Limit"=w339, "dBc Applied?"=w338) -> (w344:T3)
                n190 = Build Array (concatenate)(w347, w346) -> (w345:T1)
                n191 = Build Array (concatenate)(w342, w344) -> (w341:T1)
              }
              n192 = Build Array (concatenate)(w330, T3 {"Freq"=26500.0, "Limit"=-30.0, "dBc Applied?"=FALSE} ("Mask Table")) -> (w328:T1)
              n193 = Build Array (concatenate)(w300, T3 {"Freq"=26500.0, "Limit"=-30.0, "dBc Applied?"=FALSE} ("Mask Table")) -> (w299:T1)
            }
            frame 11103 {
              w370 = dbl[] [-30.0, -30.0, -30.0, -20.0, 0.0]
              w376 = bool[] [FALSE, FALSE, FALSE, TRUE, TRUE]
              # "dBc Applied?"
              # "Amplitude"
              n194 = Unbundle By Name(w371) -> ("BW_N"=w358:dbl)
              n195 = Multiply(x=1.5, y=w358) -> (x*y=w355:dbl)
              n196 = Subtract(x=w356, y=w355) -> (x-y=w380:dbl)
              n197 = Subtract(x=w356, y=w358) -> (x-y=w369:dbl)
              n198 = Reverse 1D Array(array=w376) -> (reversed array=w377:bool[])
              n199 = Add(x=w369, y=140.0 ("x")) -> (x+y=w368:dbl)
              n200 = Add(x=w356, y=w355) -> (x+y=w354:dbl)
              n201 = Add(x=w356, y=w358) -> (x+y=w357:dbl)
              n202 = Reverse 1D Array(array=w370) -> (reversed array=w379:dbl[])
              n203 = Build Array (concatenate)(w376, w377) -> (w375:bool[])
              n204 = Add(x=w368, y=100.0) -> (x+y=w364:dbl)
              n205 = Build Array (concatenate)(w370, w379) -> (w378:dbl[])
              n206 = Add(x=w364, y=200.0) -> (x+y=w361:dbl)
              n207 = Decrement(x=w364) -> (x-1=w366:dbl)
              n208 = Increment(x=w361) -> (x+1=w362:dbl)
              n209 = Add(x=w361, y=100.0) -> (x+y=w359:dbl)
              n210 = Build Array(w380, w369, w368, w366, w364, w361, w362, w359, w357, w354) -> (w365:dbl[])
              n211 = for {
                tunnel: w365 -> [w397] mode=indexing
                tunnel: w378 -> [w396] mode=indexing
                tunnel: w375 -> [w395] mode=indexing
                shift-right: [w392] -> w373
                shift-left: T1 [{"Freq"=0.0, "Limit"=-30.0, "dBc Applied?"=FALSE}] ("value") -> [w394]
                n212 = Bundle By Name(cluster=T3 {"Freq"=0.0, "Limit"=0.0, "dBc Applied?"=FALSE} ("Mask Table"), "Freq"=w397, "Limit"=w396, "dBc Applied?"=w395) -> (w393:T3)
                n213 = Build Array (concatenate)(w394, w393) -> (w392:T1)
              }
              n214 = Build Array (concatenate)(w373, T3 {"Freq"=26500.0, "Limit"=-30.0, "dBc Applied?"=FALSE} ("Mask Table")) -> (w352:T1)
              n215 = for {
                tunnel: w352 -> [w383] mode=indexing
                tunnel: [w382] -> w351 mode=indexing
                n216 = Unbundle By Name(w383) -> ("Limit"=w386:dbl)
                n217 = Equal?(x=w386, y=-20.0) -> (x = y?=w384:bool)
                n218 = case shown="True" w384 {
                  tunnel: w383 -> [w387 w391]
                  tunnel: [w387 w388] -> w382
                  frame False {
                  }
                  frame True {
                    n219 = Bundle By Name(cluster=w391, "Limit"=-30.0, "dBc Applied?"=FALSE) -> (w388:T3)
                  }
                }
              }
            }
            frame 104 {
              w418 = dbl[] [-30.0, -30.0, -30.0, -20.0, 0.0]
              w424 = bool[] [FALSE, FALSE, FALSE, TRUE, TRUE]
              # "dBc Applied?"
              # "Amplitude"
              n220 = Unbundle By Name(w419) -> ("BW_N"=w406:dbl)
              n221 = Multiply(x=1.5, y=w406) -> (x*y=w403:dbl)
              n222 = Subtract(x=w404, y=w403) -> (x-y=w428:dbl)
              n223 = Subtract(x=w404, y=w406) -> (x-y=w417:dbl)
              n224 = Add(x=w417, y=120.0 ("x")) -> (x+y=w416:dbl)
              n225 = Add(x=w404, y=w403) -> (x+y=w402:dbl)
              n226 = Add(x=w404, y=w406) -> (x+y=w405:dbl)
              n227 = Add(x=w416, y=120.0) -> (x+y=w412:dbl)
              n228 = Add(x=w412, y=240.0) -> (x+y=w409:dbl)
              n229 = Decrement(x=w412) -> (x-1=w414:dbl)
              n230 = Increment(x=w409) -> (x+1=w410:dbl)
              n231 = Add(x=w409, y=120.0) -> (x+y=w407:dbl)
              n232 = Reverse 1D Array(array=w424) -> (reversed array=w425:bool[])
              n233 = Reverse 1D Array(array=w418) -> (reversed array=w427:dbl[])
              n234 = Build Array (concatenate)(w424, w425) -> (w423:bool[])
              n235 = Build Array (concatenate)(w418, w427) -> (w426:dbl[])
              n236 = Build Array(w428, w417, w416, w414, w412, w409, w410, w407, w405, w402) -> (w413:dbl[])
              n237 = for {
                tunnel: w413 -> [w445] mode=indexing
                tunnel: w426 -> [w444] mode=indexing
                tunnel: w423 -> [w443] mode=indexing
                shift-right: [w440] -> w421
                shift-left: T1 [{"Freq"=0.0, "Limit"=-30.0, "dBc Applied?"=FALSE}] ("value") -> [w442]
                n238 = Bundle By Name(cluster=T3 {"Freq"=0.0, "Limit"=0.0, "dBc Applied?"=FALSE} ("Mask Table"), "Freq"=w445, "Limit"=w444, "dBc Applied?"=w443) -> (w441:T3)
                n239 = Build Array (concatenate)(w442, w441) -> (w440:T1)
              }
              n240 = Build Array (concatenate)(w421, T3 {"Freq"=26500.0, "Limit"=-30.0, "dBc Applied?"=FALSE} ("Mask Table")) -> (w400:T1)
              n241 = for {
                tunnel: w400 -> [w431] mode=indexing
                tunnel: [w430] -> w399 mode=indexing
                n242 = Unbundle By Name(w431) -> ("Limit"=w434:dbl)
                n243 = Equal?(x=w434, y=-20.0) -> (x = y?=w432:bool)
                n244 = case shown="True" w432 {
                  tunnel: w431 -> [w435 w439]
                  tunnel: [w435 w436] -> w430
                  frame False {
                  }
                  frame True {
                    n245 = Bundle By Name(cluster=w439, "Limit"=-30.0, "dBc Applied?"=FALSE) -> (w436:T3)
                  }
                }
              }
            }
            frame 11104 {
              w466 = dbl[] [-30.0, -30.0, -30.0, -20.0, 0.0]
              w472 = bool[] [FALSE, FALSE, FALSE, TRUE, TRUE]
              # "dBc Applied?"
              # "Amplitude"
              n246 = Unbundle By Name(w467) -> ("BW_N"=w454:dbl)
              n247 = Multiply(x=1.5, y=w454) -> (x*y=w451:dbl)
              n248 = Subtract(x=w452, y=w451) -> (x-y=w476:dbl)
              n249 = Subtract(x=w452, y=w454) -> (x-y=w465:dbl)
              n250 = Add(x=w465, y=40.0 ("x")) -> (x+y=w464:dbl)
              n251 = Add(x=w452, y=w451) -> (x+y=w450:dbl)
              n252 = Add(x=w452, y=w454) -> (x+y=w453:dbl)
              n253 = Add(x=w464, y=120.0) -> (x+y=w460:dbl)
              n254 = Add(x=w460, y=240.0) -> (x+y=w457:dbl)
              n255 = Decrement(x=w460) -> (x-1=w462:dbl)
              n256 = Increment(x=w457) -> (x+1=w458:dbl)
              n257 = Add(x=w457, y=120.0) -> (x+y=w455:dbl)
              n258 = Reverse 1D Array(array=w472) -> (reversed array=w473:bool[])
              n259 = Reverse 1D Array(array=w466) -> (reversed array=w475:dbl[])
              n260 = Build Array (concatenate)(w472, w473) -> (w471:bool[])
              n261 = Build Array (concatenate)(w466, w475) -> (w474:dbl[])
              n262 = Build Array(w476, w465, w464, w462, w460, w457, w458, w455, w453, w450) -> (w461:dbl[])
              n263 = for {
                tunnel: w461 -> [w493] mode=indexing
                tunnel: w474 -> [w492] mode=indexing
                tunnel: w471 -> [w491] mode=indexing
                shift-right: [w488] -> w469
                shift-left: T1 [{"Freq"=0.0, "Limit"=-30.0, "dBc Applied?"=FALSE}] ("value") -> [w490]
                n264 = Bundle By Name(cluster=T3 {"Freq"=0.0, "Limit"=0.0, "dBc Applied?"=FALSE} ("Mask Table"), "Freq"=w493, "Limit"=w492, "dBc Applied?"=w491) -> (w489:T3)
                n265 = Build Array (concatenate)(w490, w489) -> (w488:T1)
              }
              n266 = Build Array (concatenate)(w469, T3 {"Freq"=26500.0, "Limit"=-30.0, "dBc Applied?"=FALSE} ("Mask Table")) -> (w448:T1)
              n267 = for {
                tunnel: w448 -> [w479] mode=indexing
                tunnel: [w478] -> w447 mode=indexing
                n268 = Unbundle By Name(w479) -> ("Limit"=w482:dbl)
                n269 = Equal?(x=w482, y=-20.0) -> (x = y?=w480:bool)
                n270 = case shown="True" w480 {
                  tunnel: w479 -> [w483 w487]
                  tunnel: [w483 w484] -> w478
                  frame False {
                  }
                  frame True {
                    n271 = Bundle By Name(cluster=w487, "Limit"=-30.0, "dBc Applied?"=FALSE) -> (w484:T3)
                  }
                }
              }
            }
            frame 105 {
              w514 = dbl[] [-30.0, -30.0, -30.0, -20.0, 0.0]
              w520 = bool[] [FALSE, FALSE, FALSE, TRUE, TRUE]
              # "dBc Applied?"
              # "Amplitude"
              n272 = Unbundle By Name(w515) -> ("BW_N"=w502:dbl)
              n273 = Multiply(x=1.5, y=w502) -> (x*y=w499:dbl)
              n274 = Subtract(x=w500, y=w499) -> (x-y=w524:dbl)
              n275 = Subtract(x=w500, y=w502) -> (x-y=w513:dbl)
              n276 = Add(x=w513, y=60.0 ("x")) -> (x+y=w512:dbl)
              n277 = Add(x=w500, y=w499) -> (x+y=w498:dbl)
              n278 = Add(x=w500, y=w502) -> (x+y=w501:dbl)
              n279 = Add(x=w512, y=140.0) -> (x+y=w508:dbl)
              n280 = Add(x=w508, y=280.0) -> (x+y=w505:dbl)
              n281 = Decrement(x=w508) -> (x-1=w510:dbl)
              n282 = Increment(x=w505) -> (x+1=w506:dbl)
              n283 = Add(x=w505, y=140.0) -> (x+y=w503:dbl)
              n284 = Reverse 1D Array(array=w520) -> (reversed array=w521:bool[])
              n285 = Reverse 1D Array(array=w514) -> (reversed array=w523:dbl[])
              n286 = Build Array (concatenate)(w520, w521) -> (w519:bool[])
              n287 = Build Array (concatenate)(w514, w523) -> (w522:dbl[])
              n288 = Build Array(w524, w513, w512, w510, w508, w505, w506, w503, w501, w498) -> (w509:dbl[])
              n289 = for {
                tunnel: w509 -> [w541] mode=indexing
                tunnel: w522 -> [w540] mode=indexing
                tunnel: w519 -> [w539] mode=indexing
                shift-right: [w536] -> w517
                shift-left: T1 [{"Freq"=0.0, "Limit"=-30.0, "dBc Applied?"=FALSE}] ("value") -> [w538]
                n290 = Bundle By Name(cluster=T3 {"Freq"=0.0, "Limit"=0.0, "dBc Applied?"=FALSE} ("Mask Table"), "Freq"=w541, "Limit"=w540, "dBc Applied?"=w539) -> (w537:T3)
                n291 = Build Array (concatenate)(w538, w537) -> (w536:T1)
              }
              n292 = Build Array (concatenate)(w517, T3 {"Freq"=26500.0, "Limit"=-30.0, "dBc Applied?"=FALSE} ("Mask Table")) -> (w496:T1)
              n293 = for {
                tunnel: w496 -> [w527] mode=indexing
                tunnel: [w526] -> w495 mode=indexing
                n294 = Unbundle By Name(w527) -> ("Limit"=w530:dbl)
                n295 = Equal?(x=w530, y=-20.0) -> (x = y?=w528:bool)
                n296 = case shown="True" w528 {
                  tunnel: w527 -> [w531 w535]
                  tunnel: [w531 w532] -> w526
                  frame False {
                  }
                  frame True {
                    n297 = Bundle By Name(cluster=w535, "Limit"=-30.0, "dBc Applied?"=FALSE) -> (w532:T3)
                  }
                }
              }
            }
            frame 11106 {
              w562 = dbl[] [-30.0, -30.0, -30.0, -20.0, 0.0]
              w568 = bool[] [FALSE, FALSE, FALSE, TRUE, TRUE]
              # "dBc Applied?"
              # "Amplitude"
              n298 = Unbundle By Name(w563) -> ("BW_N"=w550:dbl)
              n299 = Multiply(x=1.5, y=w550) -> (x*y=w547:dbl)
              n300 = Subtract(x=w548, y=w547) -> (x-y=w572:dbl)
              n301 = Subtract(x=w548, y=w550) -> (x-y=w561:dbl)
              n302 = Add(x=w561, y=20.0 ("x")) -> (x+y=w560:dbl)
              n303 = Add(x=w548, y=w547) -> (x+y=w546:dbl)
              n304 = Add(x=w548, y=w550) -> (x+y=w549:dbl)
              n305 = Add(x=w560, y=140.0) -> (x+y=w556:dbl)
              n306 = Add(x=w556, y=280.0) -> (x+y=w553:dbl)
              n307 = Decrement(x=w556) -> (x-1=w558:dbl)
              n308 = Increment(x=w553) -> (x+1=w554:dbl)
              n309 = Add(x=w553, y=140.0) -> (x+y=w551:dbl)
              n310 = Reverse 1D Array(array=w568) -> (reversed array=w569:bool[])
              n311 = Reverse 1D Array(array=w562) -> (reversed array=w571:dbl[])
              n312 = Build Array (concatenate)(w568, w569) -> (w567:bool[])
              n313 = Build Array (concatenate)(w562, w571) -> (w570:dbl[])
              n314 = Build Array(w572, w561, w560, w558, w556, w553, w554, w551, w549, w546) -> (w557:dbl[])
              n315 = for {
                tunnel: w557 -> [w589] mode=indexing
                tunnel: w570 -> [w588] mode=indexing
                tunnel: w567 -> [w587] mode=indexing
                shift-right: [w584] -> w565
                shift-left: T1 [{"Freq"=0.0, "Limit"=-30.0, "dBc Applied?"=FALSE}] ("value") -> [w586]
                n316 = Bundle By Name(cluster=T3 {"Freq"=0.0, "Limit"=0.0, "dBc Applied?"=FALSE} ("Mask Table"), "Freq"=w589, "Limit"=w588, "dBc Applied?"=w587) -> (w585:T3)
                n317 = Build Array (concatenate)(w586, w585) -> (w584:T1)
              }
              n318 = Build Array (concatenate)(w565, T3 {"Freq"=26500.0, "Limit"=-30.0, "dBc Applied?"=FALSE} ("Mask Table")) -> (w544:T1)
              n319 = for {
                tunnel: w544 -> [w575] mode=indexing
                tunnel: [w574] -> w543 mode=indexing
                n320 = Unbundle By Name(w575) -> ("Limit"=w578:dbl)
                n321 = Equal?(x=w578, y=-20.0) -> (x = y?=w576:bool)
                n322 = case shown="True" w576 {
                  tunnel: w575 -> [w579 w583]
                  tunnel: [w579 w580] -> w574
                  frame False {
                  }
                  frame True {
                    n323 = Bundle By Name(cluster=w583, "Limit"=-30.0, "dBc Applied?"=FALSE) -> (w580:T3)
                  }
                }
              }
            }
            frame 1099 {
              w615 = dbl[] [-30.0, -30.0, -30.0, -20.0, 0.0]
              w624 = bool[] [FALSE, FALSE, FALSE, TRUE, TRUE]
              # "dBc Applied?"
              # "Amplitude"
              n324 = Unbundle By Name(w617) -> ("BW_M"=w597:dbl)
              n325 = Unbundle By Name(w617) -> ("BW_N"=w598:dbl)
              n326 = Subtract(x=w598, y=w597) -> (x-y=w596:dbl)
              n327 = Multiply(x=1.5, y=w598) -> (x*y=w606:dbl)
              n328 = Multiply(x=w598, y=0.5) -> (x*y=w599:dbl)
              n329 = Multiply(x=w596, y=3.0) -> (x*y=w594:dbl)
              n330 = Increment(x=w599) -> (x+1=w613:dbl)
              n331 = Subtract(x=w607, y=w606) -> (x-y=w628:dbl)
              n332 = Subtract(x=w607, y=w598) -> (x-y=w614:dbl)
              n333 = Add(x=w607, y=w606) -> (x+y=w608:dbl)
              n334 = Add(x=w607, y=w598) -> (x+y=w610:dbl)
              n335 = Subtract(x=w607, y=w613) -> (x-y=w612:dbl)
              n336 = Subtract(x=w607, y=w599) -> (x-y=w611:dbl)
              n337 = Add(x=w607, y=w594) -> (x+y=w605:dbl)
              n338 = Add(x=w614, y=10.0 ("x")) -> (x+y=w616:dbl)
              n339 = Subtract(x=w610, y=30.0) -> (x-y=w609:dbl)
              n340 = Increment(x=w605) -> (x+1=w604:dbl)
              n341 = Reverse 1D Array(array=w624) -> (reversed array=w625:bool[])
              n342 = Build Array(w628, w614, w616, w612, w611) -> (w621:dbl[])
              n343 = Build Array(w608, w610, w609, w604, w605) -> (w603:dbl[])
              n344 = Reverse 1D Array(array=w615) -> (reversed array=w627:dbl[])
              n345 = Build Array (concatenate)(w624, w625) -> (w623:bool[])
              n346 = Reverse 1D Array(array=w603) -> (reversed array=w602:dbl[])
              n347 = Build Array (concatenate)(w615, w627) -> (w626:dbl[])
              n348 = Build Array (concatenate)(w621, w602) -> (w620:dbl[])
              n349 = for {
                tunnel: w620 -> [w645] mode=indexing
                tunnel: w626 -> [w644] mode=indexing
                tunnel: w623 -> [w643] mode=indexing
                shift-right: [w640] -> w619
                shift-left: T1 [{"Freq"=0.0, "Limit"=-30.0, "dBc Applied?"=FALSE}] ("value") -> [w642]
                n350 = Bundle By Name(cluster=T3 {"Freq"=0.0, "Limit"=0.0, "dBc Applied?"=FALSE} ("Mask Table"), "Freq"=w645, "Limit"=w644, "dBc Applied?"=w643) -> (w641:T3)
                n351 = Build Array (concatenate)(w642, w641) -> (w640:T1)
              }
              n352 = Build Array (concatenate)(w619, T3 {"Freq"=26500.0, "Limit"=-30.0, "dBc Applied?"=FALSE} ("Mask Table")) -> (w592:T1)
              n353 = for {
                tunnel: w592 -> [w631] mode=indexing
                tunnel: [w630] -> w591 mode=indexing
                n354 = Unbundle By Name(w631) -> ("Limit"=w634:dbl)
                n355 = Equal?(x=w634, y=-20.0) -> (x = y?=w632:bool)
                n356 = case shown="True" w632 {
                  tunnel: w631 -> [w635 w639]
                  tunnel: [w635 w636] -> w630
                  frame False {
                  }
                  frame True {
                    n357 = Bundle By Name(cluster=w639, "Limit"=-30.0, "dBc Applied?"=FALSE) -> (w636:T3)
                  }
                }
              }
            }
            frame 93, 1095 {
              w671 = dbl[] [-30.0, -30.0, -30.0, -20.0, 0.0]
              w680 = bool[] [FALSE, FALSE, FALSE, TRUE, TRUE]
              # "dBc Applied?"
              # "Amplitude"
              n358 = Unbundle By Name(w673) -> ("BW_M"=w650:dbl)
              n359 = Unbundle By Name(w673) -> ("BW_N"=w651:dbl)
              n360 = Subtract(x=w651, y=w650) -> (x-y=w654:dbl)
              n361 = Multiply(x=1.5, y=w651) -> (x*y=w659:dbl)
              n362 = Multiply(x=w651, y=0.5) -> (x*y=w652:dbl)
              n363 = Subtract(x=w651, y=w650) -> (x-y=w649:dbl)
              n364 = Increment(x=w652) -> (x+1=w668:dbl)
              n365 = Multiply(x=w650, y=0.5) -> (x*y=w660:dbl)
              n366 = Multiply(x=w654, y=0.5) -> (x*y=w669:dbl)
              n367 = Subtract(x=w662, y=w659) -> (x-y=w684:dbl)
              n368 = Subtract(x=w662, y=w651) -> (x-y=w670:dbl)
              n369 = Add(x=w662, y=w659) -> (x+y=w663:dbl)
              n370 = Add(x=w662, y=w651) -> (x+y=w665:dbl)
              n371 = Subtract(x=w662, y=w668) -> (x-y=w667:dbl)
              n372 = Subtract(x=w662, y=w652) -> (x-y=w666:dbl)
              n373 = Add(x=w662, y=w649) -> (x+y=w658:dbl)
              n374 = Add(x=w670, y=w669) -> (x+y=w672:dbl)
              n375 = Subtract(x=w665, y=w660) -> (x-y=w664:dbl)
              n376 = Increment(x=w658) -> (x+1=w657:dbl)
              n377 = Reverse 1D Array(array=w680) -> (reversed array=w681:bool[])
              n378 = Build Array(w684, w670, w672, w667, w666) -> (w677:dbl[])
              n379 = Build Array(w663, w665, w664, w657, w658) -> (w656:dbl[])
              n380 = Reverse 1D Array(array=w671) -> (reversed array=w683:dbl[])
              n381 = Build Array (concatenate)(w680, w681) -> (w679:bool[])
              n382 = Reverse 1D Array(array=w656) -> (reversed array=w655:dbl[])
              n383 = Build Array (concatenate)(w671, w683) -> (w682:dbl[])
              n384 = Build Array (concatenate)(w677, w655) -> (w676:dbl[])
              n385 = for {
                tunnel: w676 -> [w702] mode=indexing
                tunnel: w682 -> [w701] mode=indexing
                tunnel: w679 -> [w700] mode=indexing
                shift-right: [w697] -> w675
                shift-left: T1 [{"Freq"=0.0, "Limit"=-30.0, "dBc Applied?"=FALSE}] ("value") -> [w699]
                n386 = Bundle By Name(cluster=T3 {"Freq"=0.0, "Limit"=0.0, "dBc Applied?"=FALSE} ("Mask Table"), "Freq"=w702, "Limit"=w701, "dBc Applied?"=w700) -> (w698:T3)
                n387 = Build Array (concatenate)(w699, w698) -> (w697:T1)
              }
              n388 = Build Array (concatenate)(w675, T3 {"Freq"=26500.0, "Limit"=-30.0, "dBc Applied?"=FALSE} ("Mask Table")) -> (w648:T1)
              n389 = for {
                tunnel: w648 -> [w688] mode=indexing
                tunnel: [w687] -> w647 mode=indexing
                n390 = Unbundle By Name(w688) -> ("Limit"=w691:dbl)
                n391 = Equal?(x=w691, y=-20.0) -> (x = y?=w689:bool)
                n392 = case shown="True" w689 {
                  tunnel: w688 -> [w692 w696]
                  tunnel: [w692 w693] -> w687
                  frame False {
                  }
                  frame True {
                    n393 = Bundle By Name(cluster=w696, "Limit"=-30.0, "dBc Applied?"=FALSE) -> (w693:T3)
                  }
                }
              }
            }
          }
        }
        frame "Case 3" {
          n394 = case shown="91" w705 {
            tunnel: [_ w741 w792 w843 w894 w945 w996 w1047 w1098] -> w708
            tunnel: w707 -> [_ w740 w791 w842 w893 w944 w995 w1046 w1097]
            tunnel: w706 -> [_ w718 w773 w824 w875 w926 w977 w1028 w1079]
            tunnel: [_ w709 w760 w811 w862 w913 w964 w1015 w1066] -> w704
            frame 0, Default {
            }
            frame 91 {
              w714 = T1 [{"Freq"=0.0, "Limit"=-30.0, "dBc Applied?"=FALSE}] ("value")
              # "dBc Applied?"
              # "Amplitude"
              # "dBc Applied?"
              # "Amplitude"
              n395 = Unbundle By Name(w740) -> ("BW_N"=w715:dbl)
              n396 = Multiply(x=1.5, y=w715) -> (x*y=w717:dbl)
              n397 = Multiply(x=w715, y=0.5) -> (x*y=w720:dbl)
              n398 = Multiply(x=w715, y=0.25) -> (x*y=w731:dbl)
              n399 = Multiply(x=w715, y=0.125) -> (x*y=w727:dbl)
              n400 = Increment(x=w720) -> (x+1=w735:dbl)
              n401 = Subtract(x=w718, y=w717) -> (x-y=w745:dbl)
              n402 = Subtract(x=w718, y=w715) -> (x-y=w739:dbl)
              n403 = Subtract(x=w718, y=w735) -> (x-y=w734:dbl)
              n404 = Subtract(x=w718, y=w720) -> (x-y=w732:dbl)
              n405 = Subtract(x=w718, y=w731) -> (x-y=w730:dbl)
              n406 = Subtract(x=w718, y=w727) -> (x-y=w726:dbl)
              n407 = Subtract(x=w718, y=0.0) -> (x-y=w723:dbl)
              n408 = Add(x=w718, y=w720) -> (x+y=w722:dbl)
              n409 = Add(x=w718, y=w715) -> (x+y=w719:dbl)
              n410 = Add(x=w718, y=w717) -> (x+y=w716:dbl)
              n411 = Increment(x=w730) -> (x+1=w729:dbl)
              n412 = Decrement(x=w723) -> (x-1=w724:dbl)
              n413 = Increment(x=w722) -> (x+1=w721:dbl)
              n414 = Build Array(w745, w739, w734, w732, w730, w729, w726, w724, w723, w722, w721, w719, w716) -> (w744:dbl[])
              n415 = for {
                tunnel: w744 -> [w749] mode=indexing
                tunnel: dbl[] [-30.0, -30.0, -20.0, 0.0, 0.0, -20.0, -23.0, -20.0, 0.0, 0.0, -20.0, -30.0, -30.0] -> [w758] mode=indexing
                tunnel: bool[] [FALSE, FALSE, TRUE, TRUE, TRUE, TRUE, TRUE, TRUE, TRUE, TRUE, TRUE, FALSE, FALSE] -> [w757] mode=indexing
                shift-right: [w754] -> w743
                shift-left: w714 -> [w756]
                shift-right: [w750] -> w710
                shift-left: w714 -> [w751]
                tunnel: dbl[] [-30.0, -30.0, -30.0, 0.0, 0.0, -20.0, -23.0, -20.0, 0.0, 0.0, -30.0, -30.0, -30.0] -> [w748] mode=indexing
                tunnel: bool[] [FALSE, FALSE, FALSE, TRUE, TRUE, TRUE, TRUE, TRUE, TRUE, TRUE, FALSE, FALSE, FALSE] -> [w747] mode=indexing
                n416 = Bundle By Name(cluster=T3 {"Freq"=0.0, "Limit"=0.0, "dBc Applied?"=FALSE} ("Mask Table"), "Freq"=w749, "Limit"=w748, "dBc Applied?"=w747) -> (w753:T3)
                n417 = Bundle By Name(cluster=T3 {"Freq"=0.0, "Limit"=0.0, "dBc Applied?"=FALSE} ("Mask Table"), "Freq"=w749, "Limit"=w758, "dBc Applied?"=w757) -> (w755:T3)
                n418 = Build Array (concatenate)(w751, w753) -> (w750:T1)
                n419 = Build Array (concatenate)(w756, w755) -> (w754:T1)
              }
              n420 = Build Array (concatenate)(w743, T3 {"Freq"=26500.0, "Limit"=-30.0, "dBc Applied?"=FALSE} ("Mask Table")) -> (w741:T1)
              n421 = Build Array (concatenate)(w710, T3 {"Freq"=26500.0, "Limit"=-30.0, "dBc Applied?"=FALSE} ("Mask Table")) -> (w709:T1)
            }
            frame 92 {
              w765 = T1 [{"Freq"=0.0, "Limit"=-30.0, "dBc Applied?"=FALSE}] ("value")
              # "dBc Applied?"
              # "Amplitude"
              # "dBc Applied?"
              # "Amplitude"
              n422 = Unbundle By Name(w791) -> ("BW_N"=w776:dbl)
              n423 = Multiply(x=1.5, y=w776) -> (x*y=w781:dbl)
              n424 = Multiply(x=w776, y=0.5) -> (x*y=w782:dbl)
              n425 = Multiply(x=w776, y=0.125) -> (x*y=w777:dbl)
              n426 = Multiply(x=w776, y=0.25) -> (x*y=w772:dbl)
              n427 = Increment(x=w782) -> (x+1=w786:dbl)
              n428 = Subtract(x=w773, y=w781) -> (x-y=w796:dbl)
              n429 = Subtract(x=w773, y=w776) -> (x-y=w790:dbl)
              n430 = Subtract(x=w773, y=w786) -> (x-y=w785:dbl)
              n431 = Subtract(x=w773, y=w782) -> (x-y=w784:dbl)
              n432 = Add(x=w773, y=w782) -> (x+y=w769:dbl)
              n433 = Subtract(x=w773, y=0.0) -> (x-y=w779:dbl)
              n434 = Add(x=w773, y=w776) -> (x+y=w767:dbl)
              n435 = Add(x=w773, y=w781) -> (x+y=w766:dbl)
              n436 = Add(x=w773, y=w777) -> (x+y=w774:dbl)
              n437 = Add(x=w773, y=w772) -> (x+y=w770:dbl)
              n438 = Increment(x=w779) -> (x+1=w778:dbl)
              n439 = Decrement(x=w770) -> (x-1=w771:dbl)
              n440 = Increment(x=w769) -> (x+1=w768:dbl)
              n441 = Build Array(w796, w790, w785, w784, w779, w778, w774, w771, w770, w769, w768, w767, w766) -> (w795:dbl[])
              n442 = for {
                tunnel: w795 -> [w800] mode=indexing
                tunnel: dbl[] [-30.0, -30.0, -20.0, 0.0, 0.0, -20.0, -23.0, -20.0, 0.0, 0.0, -20.0, -30.0, -30.0] -> [w809] mode=indexing
                tunnel: bool[] [FALSE, FALSE, TRUE, TRUE, TRUE, TRUE, TRUE, TRUE, TRUE, TRUE, TRUE, FALSE, FALSE] -> [w808] mode=indexing
                shift-right: [w805] -> w794
                shift-left: w765 -> [w807]
                shift-right: [w801] -> w761
                shift-left: w765 -> [w802]
                tunnel: dbl[] [-30.0, -30.0, -30.0, 0.0, 0.0, -20.0, -23.0, -20.0, 0.0, 0.0, -30.0, -30.0, -30.0] -> [w799] mode=indexing
                tunnel: bool[] [FALSE, FALSE, FALSE, TRUE, TRUE, TRUE, TRUE, TRUE, TRUE, TRUE, FALSE, FALSE, FALSE] -> [w798] mode=indexing
                n443 = Bundle By Name(cluster=T3 {"Freq"=0.0, "Limit"=0.0, "dBc Applied?"=FALSE} ("Mask Table"), "Freq"=w800, "Limit"=w799, "dBc Applied?"=w798) -> (w804:T3)
                n444 = Bundle By Name(cluster=T3 {"Freq"=0.0, "Limit"=0.0, "dBc Applied?"=FALSE} ("Mask Table"), "Freq"=w800, "Limit"=w809, "dBc Applied?"=w808) -> (w806:T3)
                n445 = Build Array (concatenate)(w802, w804) -> (w801:T1)
                n446 = Build Array (concatenate)(w807, w806) -> (w805:T1)
              }
              n447 = Build Array (concatenate)(w794, T3 {"Freq"=26500.0, "Limit"=-30.0, "dBc Applied?"=FALSE} ("Mask Table")) -> (w792:T1)
              n448 = Build Array (concatenate)(w761, T3 {"Freq"=26500.0, "Limit"=-30.0, "dBc Applied?"=FALSE} ("Mask Table")) -> (w760:T1)
            }
            frame 97 {
              w816 = T1 [{"Freq"=0.0, "Limit"=-30.0, "dBc Applied?"=FALSE}] ("value")
              # "dBc Applied?"
              # "Amplitude"
              # "dBc Applied?"
              # "Amplitude"
              n449 = Unbundle By Name(w842) -> ("BW_N"=w834:dbl)
              n450 = Multiply(x=1.5, y=w834) -> (x*y=w835:dbl)
              n451 = Multiply(x=w834, y=0.5) -> (x*y=w836:dbl)
              n452 = Multiply(x=w834, y=0.125) -> ()  [unwired: 1 out]
              n453 = Multiply(x=w834, y=0.25) -> ()  [unwired: 1 out]
              n454 = Increment(x=w836) -> (x+1=w839:dbl)
              n455 = Subtract(x=w824, y=w835) -> (x-y=w847:dbl)
              n456 = Subtract(x=w824, y=w834) -> (x-y=w841:dbl)
              n457 = Subtract(x=w824, y=w839) -> (x-y=w838:dbl)
              n458 = Subtract(x=w824, y=w836) -> (x-y=w828:dbl)
              n459 = Add(x=w824, y=w836) -> (x+y=w832:dbl)
              n460 = Add(x=w824, y=w834) -> (x+y=w830:dbl)
              n461 = Add(x=w824, y=w835) -> (x+y=w829:dbl)
              n462 = Subtract(x=w824, y=50.0) -> (x-y=w822:dbl)
              n463 = Add(x=w828, y=20.0) -> (x+y=w826:dbl)
              n464 = Add(x=w822, y=10.0) -> (x+y=w819:dbl)
              n465 = Increment(x=w832) -> (x+1=w831:dbl)
              n466 = Increment(x=w826) -> (x+1=w825:dbl)
              n467 = Decrement(x=w819) -> (x-1=w820:dbl)
              n468 = Build Array(w847, w841, w838, w828, w826, w825, w822, w820, w819, w832, w831, w830, w829) -> (w846:dbl[])
              n469 = for {
                tunnel: w846 -> [w851] mode=indexing
                tunnel: dbl[] [-30.0, -30.0, -20.0, 0.0, 0.0, -20.0, -23.0, -20.0, 0.0, 0.0, -20.0, -30.0, -30.0] -> [w860] mode=indexing
                tunnel: bool[] [FALSE, FALSE, TRUE, TRUE, TRUE, TRUE, TRUE, TRUE, TRUE, TRUE, TRUE, FALSE, FALSE] -> [w859] mode=indexing
                shift-right: [w856] -> w845
                shift-left: w816 -> [w858]
                shift-right: [w852] -> w812
                shift-left: w816 -> [w853]
                tunnel: dbl[] [-30.0, -30.0, -30.0, 0.0, 0.0, -20.0, -23.0, -20.0, 0.0, 0.0, -30.0, -30.0, -30.0] -> [w850] mode=indexing
                tunnel: bool[] [FALSE, FALSE, FALSE, TRUE, TRUE, TRUE, TRUE, TRUE, TRUE, TRUE, FALSE, FALSE, FALSE] -> [w849] mode=indexing
                n470 = Bundle By Name(cluster=T3 {"Freq"=0.0, "Limit"=0.0, "dBc Applied?"=FALSE} ("Mask Table"), "Freq"=w851, "Limit"=w860, "dBc Applied?"=w859) -> (w857:T3)
                n471 = Bundle By Name(cluster=T3 {"Freq"=0.0, "Limit"=0.0, "dBc Applied?"=FALSE} ("Mask Table"), "Freq"=w851, "Limit"=w850, "dBc Applied?"=w849) -> (w855:T3)
                n472 = Build Array (concatenate)(w858, w857) -> (w856:T1)
                n473 = Build Array (concatenate)(w853, w855) -> (w852:T1)
              }
              n474 = Build Array (concatenate)(w845, T3 {"Freq"=26500.0, "Limit"=-30.0, "dBc Applied?"=FALSE} ("Mask Table")) -> (w843:T1)
              n475 = Build Array (concatenate)(w812, T3 {"Freq"=26500.0, "Limit"=-30.0, "dBc Applied?"=FALSE} ("Mask Table")) -> (w811:T1)
            }
            frame 98 {
              w867 = T1 [{"Freq"=0.0, "Limit"=-30.0, "dBc Applied?"=FALSE}] ("value")
              # "dBc Applied?"
              # "Amplitude"
              # "dBc Applied?"
              # "Amplitude"
              n476 = Unbundle By Name(w893) -> ("BW_N"=w885:dbl)
              n477 = Multiply(x=1.5, y=w885) -> (x*y=w886:dbl)
              n478 = Multiply(x=w885, y=0.5) -> (x*y=w887:dbl)
              n479 = Multiply(x=w885, y=0.125) -> ()  [unwired: 1 out]
              n480 = Multiply(x=w885, y=0.25) -> ()  [unwired: 1 out]
              n481 = Increment(x=w887) -> (x+1=w890:dbl)
              n482 = Subtract(x=w875, y=w886) -> (x-y=w898:dbl)
              n483 = Subtract(x=w875, y=w885) -> (x-y=w892:dbl)
              n484 = Subtract(x=w875, y=w890) -> (x-y=w889:dbl)
              n485 = Subtract(x=w875, y=w887) -> (x-y=w879:dbl)
              n486 = Add(x=w875, y=w887) -> (x+y=w883:dbl)
              n487 = Add(x=w875, y=w885) -> (x+y=w881:dbl)
              n488 = Add(x=w875, y=w886) -> (x+y=w880:dbl)
              n489 = Subtract(x=w875, y=30.0) -> (x-y=w873:dbl)
              n490 = Add(x=w879, y=40.0) -> (x+y=w877:dbl)
              n491 = Add(x=w873, y=10.0) -> (x+y=w870:dbl)
              n492 = Increment(x=w883) -> (x+1=w882:dbl)
              n493 = Increment(x=w877) -> (x+1=w876:dbl)
              n494 = Decrement(x=w870) -> (x-1=w871:dbl)
              n495 = Build Array(w898, w892, w889, w879, w877, w876, w873, w871, w870, w883, w882, w881, w880) -> (w897:dbl[])
              n496 = for {
                tunnel: w897 -> [w902] mode=indexing
                tunnel: dbl[] [-30.0, -30.0, -20.0, 0.0, 0.0, -20.0, -23.0, -20.0, 0.0, 0.0, -20.0, -30.0, -30.0] -> [w911] mode=indexing
                tunnel: bool[] [FALSE, FALSE, TRUE, TRUE, TRUE, TRUE, TRUE, TRUE, TRUE, TRUE, TRUE, FALSE, FALSE] -> [w910] mode=indexing
                shift-right: [w907] -> w896
                shift-left: w867 -> [w909]
                shift-right: [w903] -> w863
                shift-left: w867 -> [w904]
                tunnel: dbl[] [-30.0, -30.0, -30.0, 0.0, 0.0, -20.0, -23.0, -20.0, 0.0, 0.0, -30.0, -30.0, -30.0] -> [w901] mode=indexing
                tunnel: bool[] [FALSE, FALSE, FALSE, TRUE, TRUE, TRUE, TRUE, TRUE, TRUE, TRUE, FALSE, FALSE, FALSE] -> [w900] mode=indexing
                n497 = Bundle By Name(cluster=T3 {"Freq"=0.0, "Limit"=0.0, "dBc Applied?"=FALSE} ("Mask Table"), "Freq"=w902, "Limit"=w911, "dBc Applied?"=w910) -> (w908:T3)
                n498 = Bundle By Name(cluster=T3 {"Freq"=0.0, "Limit"=0.0, "dBc Applied?"=FALSE} ("Mask Table"), "Freq"=w902, "Limit"=w901, "dBc Applied?"=w900) -> (w906:T3)
                n499 = Build Array (concatenate)(w909, w908) -> (w907:T1)
                n500 = Build Array (concatenate)(w904, w906) -> (w903:T1)
              }
              n501 = Build Array (concatenate)(w896, T3 {"Freq"=26500.0, "Limit"=-30.0, "dBc Applied?"=FALSE} ("Mask Table")) -> (w894:T1)
              n502 = Build Array (concatenate)(w863, T3 {"Freq"=26500.0, "Limit"=-30.0, "dBc Applied?"=FALSE} ("Mask Table")) -> (w862:T1)
            }
            frame 99 {
              w918 = T1 [{"Freq"=0.0, "Limit"=-30.0, "dBc Applied?"=FALSE}] ("value")
              # "dBc Applied?"
              # "Amplitude"
              # "dBc Applied?"
              # "Amplitude"
              # "dBc Applied?"
              n503 = Unbundle By Name(w944) -> ("BW_N"=w936:dbl)
              n504 = Multiply(x=1.5, y=w936) -> (x*y=w937:dbl)
              n505 = Multiply(x=w936, y=0.5) -> (x*y=w938:dbl)
              n506 = Multiply(x=w936, y=0.125) -> ()  [unwired: 1 out]
              n507 = Multiply(x=w936, y=0.25) -> ()  [unwired: 1 out]
              n508 = Increment(x=w938) -> (x+1=w941:dbl)
              n509 = Subtract(x=w926, y=w937) -> (x-y=w949:dbl)
              n510 = Subtract(x=w926, y=w936) -> (x-y=w943:dbl)
              n511 = Subtract(x=w926, y=w941) -> (x-y=w940:dbl)
              n512 = Subtract(x=w926, y=w938) -> (x-y=w930:dbl)
              n513 = Add(x=w926, y=w938) -> (x+y=w934:dbl)
              n514 = Add(x=w926, y=w936) -> (x+y=w932:dbl)
              n515 = Add(x=w926, y=w937) -> (x+y=w931:dbl)
              n516 = Subtract(x=w926, y=10.0) -> (x-y=w924:dbl)
              n517 = Add(x=w930, y=60.0) -> (x+y=w928:dbl)
              n518 = Add(x=w924, y=10.0) -> (x+y=w921:dbl)
              n519 = Increment(x=w934) -> (x+1=w933:dbl)
              n520 = Increment(x=w928) -> (x+1=w927:dbl)
              n521 = Decrement(x=w921) -> (x-1=w922:dbl)
              n522 = Build Array(w949, w943, w940, w930, w928, w927, w924, w922, w921, w934, w933, w932, w931) -> (w948:dbl[])
              n523 = for {
                tunnel: w948 -> [w953] mode=indexing
                tunnel: dbl[] [-30.0, -30.0, -20.0, 0.0, 0.0, -20.0, -23.0, -20.0, 0.0, 0.0, -20.0, -30.0, -30.0] -> [w962] mode=indexing
                tunnel: bool[] [FALSE, FALSE, TRUE, TRUE, TRUE, TRUE, TRUE, TRUE, TRUE, TRUE, TRUE, FALSE, FALSE] -> [w961] mode=indexing
                shift-right: [w958] -> w947
                shift-left: w918 -> [w960]
                shift-right: [w954] -> w914
                shift-left: w918 -> [w955]
                tunnel: dbl[] [-30.0, -30.0, -30.0, 0.0, 0.0, -20.0, -23.0, -20.0, 0.0, 0.0, -30.0, -30.0, -30.0] -> [w952] mode=indexing
                tunnel: bool[] [FALSE, FALSE, FALSE, TRUE, TRUE, TRUE, TRUE, TRUE, TRUE, TRUE, FALSE, FALSE, FALSE] -> [w951] mode=indexing
                n524 = Bundle By Name(cluster=T3 {"Freq"=0.0, "Limit"=0.0, "dBc Applied?"=FALSE} ("Mask Table"), "Freq"=w953, "Limit"=w952, "dBc Applied?"=w951) -> (w957:T3)
                n525 = Bundle By Name(cluster=T3 {"Freq"=0.0, "Limit"=0.0, "dBc Applied?"=FALSE} ("Mask Table"), "Freq"=w953, "Limit"=w962, "dBc Applied?"=w961) -> (w959:T3)
                n526 = Build Array (concatenate)(w955, w957) -> (w954:T1)
                n527 = Build Array (concatenate)(w960, w959) -> (w958:T1)
              }
              n528 = Build Array (concatenate)(w914, T3 {"Freq"=26500.0, "Limit"=-30.0, "dBc Applied?"=FALSE} ("Mask Table")) -> (w913:T1)
              n529 = Build Array (concatenate)(w947, T3 {"Freq"=26500.0, "Limit"=-30.0, "dBc Applied?"=FALSE} ("Mask Table")) -> (w945:T1)
            }
            frame 1096 {
              w969 = T1 [{"Freq"=0.0, "Limit"=-30.0, "dBc Applied?"=FALSE}] ("value")
              # "dBc Applied?"
              # "Amplitude"
              # "dBc Applied?"
              # "Amplitude"
              # "dBc Applied?"
              n530 = Unbundle By Name(w995) -> ("BW_N"=w987:dbl)
              n531 = Multiply(x=1.5, y=w987) -> (x*y=w988:dbl)
              n532 = Multiply(x=w987, y=0.5) -> (x*y=w989:dbl)
              n533 = Multiply(x=w987, y=0.125) -> ()  [unwired: 1 out]
              n534 = Multiply(x=w987, y=0.25) -> ()  [unwired: 1 out]
              n535 = Increment(x=w989) -> (x+1=w992:dbl)
              n536 = Subtract(x=w977, y=w988) -> (x-y=w1000:dbl)
              n537 = Subtract(x=w977, y=w987) -> (x-y=w994:dbl)
              n538 = Subtract(x=w977, y=w992) -> (x-y=w991:dbl)
              n539 = Subtract(x=w977, y=w989) -> (x-y=w981:dbl)
              n540 = Add(x=w977, y=w989) -> (x+y=w985:dbl)
              n541 = Add(x=w977, y=w987) -> (x+y=w983:dbl)
              n542 = Add(x=w977, y=w988) -> (x+y=w982:dbl)
              n543 = Add(x=w977, y=10.0) -> (x+y=w975:dbl)
              n544 = Add(x=w981, y=80.0) -> (x+y=w979:dbl)
              n545 = Add(x=w975, y=10.0) -> (x+y=w972:dbl)
              n546 = Increment(x=w985) -> (x+1=w984:dbl)
              n547 = Increment(x=w979) -> (x+1=w978:dbl)
              n548 = Decrement(x=w972) -> (x-1=w973:dbl)
              n549 = Build Array(w1000, w994, w991, w981, w979, w978, w975, w973, w972, w985, w984, w983, w982) -> (w999:dbl[])
              n550 = for {
                tunnel: w999 -> [w1003] mode=indexing
                tunnel: dbl[] [-30.0, -30.0, -20.0, 0.0, 0.0, -20.0, -23.0, -20.0, 0.0, 0.0, -20.0, -30.0, -30.0] -> [w1013] mode=indexing
                tunnel: bool[] [FALSE, FALSE, TRUE, TRUE, TRUE, TRUE, TRUE, TRUE, TRUE, TRUE, TRUE, FALSE, FALSE] -> [w1012] mode=indexing
                shift-right: [w1009] -> w998
                shift-left: w969 -> [w1011]
                shift-right: [w1005] -> w965
                shift-left: w969 -> [w1006]
                tunnel: dbl[] [-30.0, -30.0, -30.0, 0.0, 0.0, -20.0, -23.0, -20.0, 0.0, 0.0, -30.0, -30.0, -30.0] -> [w1004] mode=indexing
                tunnel: bool[] [FALSE, FALSE, FALSE, TRUE, TRUE, TRUE, TRUE, TRUE, TRUE, TRUE, FALSE, FALSE, FALSE] -> [w1002] mode=indexing
                n551 = Bundle By Name(cluster=T3 {"Freq"=0.0, "Limit"=0.0, "dBc Applied?"=FALSE} ("Mask Table"), "Freq"=w1003, "Limit"=w1004, "dBc Applied?"=w1002) -> (w1008:T3)
                n552 = Bundle By Name(cluster=T3 {"Freq"=0.0, "Limit"=0.0, "dBc Applied?"=FALSE} ("Mask Table"), "Freq"=w1003, "Limit"=w1013, "dBc Applied?"=w1012) -> (w1010:T3)
                n553 = Build Array (concatenate)(w1006, w1008) -> (w1005:T1)
                n554 = Build Array (concatenate)(w1011, w1010) -> (w1009:T1)
              }
              n555 = Build Array (concatenate)(w965, T3 {"Freq"=26500.0, "Limit"=-30.0, "dBc Applied?"=FALSE} ("Mask Table")) -> (w964:T1)
              n556 = Build Array (concatenate)(w998, T3 {"Freq"=26500.0, "Limit"=-30.0, "dBc Applied?"=FALSE} ("Mask Table")) -> (w996:T1)
            }
            frame 1097 {
              w1020 = T1 [{"Freq"=0.0, "Limit"=-30.0, "dBc Applied?"=FALSE}] ("value")
              # "dBc Applied?"
              # "Amplitude"
              # "dBc Applied?"
              # "Amplitude"
              # "dBc Applied?"
              n557 = Unbundle By Name(w1046) -> ("BW_N"=w1038:dbl)
              n558 = Multiply(x=1.5, y=w1038) -> (x*y=w1039:dbl)
              n559 = Multiply(x=w1038, y=0.5) -> (x*y=w1040:dbl)
              n560 = Multiply(x=w1038, y=0.125) -> ()  [unwired: 1 out]
              n561 = Multiply(x=w1038, y=0.25) -> ()  [unwired: 1 out]
              n562 = Increment(x=w1040) -> (x+1=w1043:dbl)
              n563 = Subtract(x=w1028, y=w1039) -> (x-y=w1051:dbl)
              n564 = Subtract(x=w1028, y=w1038) -> (x-y=w1045:dbl)
              n565 = Subtract(x=w1028, y=w1043) -> (x-y=w1042:dbl)
              n566 = Subtract(x=w1028, y=w1040) -> (x-y=w1032:dbl)
              n567 = Add(x=w1028, y=w1040) -> (x+y=w1036:dbl)
              n568 = Add(x=w1028, y=w1038) -> (x+y=w1034:dbl)
              n569 = Add(x=w1028, y=w1039) -> (x+y=w1033:dbl)
              n570 = Add(x=w1028, y=30.0) -> (x+y=w1026:dbl)
              n571 = Add(x=w1032, y=100.0) -> (x+y=w1030:dbl)
              n572 = Add(x=w1026, y=10.0) -> (x+y=w1023:dbl)
              n573 = Increment(x=w1036) -> (x+1=w1035:dbl)
              n574 = Increment(x=w1030) -> (x+1=w1029:dbl)
              n575 = Decrement(x=w1023) -> (x-1=w1024:dbl)
              n576 = Build Array(w1051, w1045, w1042, w1032, w1030, w1029, w1026, w1024, w1023, w1036, w1035, w1034, w1033) -> (w1050:dbl[])
              n577 = for {
                tunnel: w1050 -> [w1055] mode=indexing
                tunnel: dbl[] [-30.0, -30.0, -20.0, 0.0, 0.0, -20.0, -23.0, -20.0, 0.0, 0.0, -20.0, -30.0, -30.0] -> [w1064] mode=indexing
                tunnel: bool[] [FALSE, FALSE, TRUE, TRUE, TRUE, TRUE, TRUE, TRUE, TRUE, TRUE, TRUE, FALSE, FALSE] -> [w1063] mode=indexing
                shift-right: [w1060] -> w1049
                shift-left: w1020 -> [w1062]
                shift-right: [w1056] -> w1016
                shift-left: w1020 -> [w1057]
                tunnel: dbl[] [-30.0, -30.0, -30.0, 0.0, 0.0, -20.0, -23.0, -20.0, 0.0, 0.0, -30.0, -30.0, -30.0] -> [w1054] mode=indexing
                tunnel: bool[] [FALSE, FALSE, FALSE, TRUE, TRUE, TRUE, TRUE, TRUE, TRUE, TRUE, FALSE, FALSE, FALSE] -> [w1053] mode=indexing
                n578 = Bundle By Name(cluster=T3 {"Freq"=0.0, "Limit"=0.0, "dBc Applied?"=FALSE} ("Mask Table"), "Freq"=w1055, "Limit"=w1064, "dBc Applied?"=w1063) -> (w1061:T3)
                n579 = Bundle By Name(cluster=T3 {"Freq"=0.0, "Limit"=0.0, "dBc Applied?"=FALSE} ("Mask Table"), "Freq"=w1055, "Limit"=w1054, "dBc Applied?"=w1053) -> (w1059:T3)
                n580 = Build Array (concatenate)(w1062, w1061) -> (w1060:T1)
                n581 = Build Array (concatenate)(w1057, w1059) -> (w1056:T1)
              }
              n582 = Build Array (concatenate)(w1016, T3 {"Freq"=26500.0, "Limit"=-30.0, "dBc Applied?"=FALSE} ("Mask Table")) -> (w1015:T1)
              n583 = Build Array (concatenate)(w1049, T3 {"Freq"=26500.0, "Limit"=-30.0, "dBc Applied?"=FALSE} ("Mask Table")) -> (w1047:T1)
            }
            frame 1098 {
              w1071 = T1 [{"Freq"=0.0, "Limit"=-30.0, "dBc Applied?"=FALSE}] ("value")
              # "dBc Applied?"
              # "Amplitude"
              # "dBc Applied?"
              # "Amplitude"
              n584 = Unbundle By Name(w1097) -> ("BW_N"=w1089:dbl)
              n585 = Multiply(x=1.5, y=w1089) -> (x*y=w1090:dbl)
              n586 = Multiply(x=w1089, y=0.5) -> (x*y=w1091:dbl)
              n587 = Multiply(x=w1089, y=0.125) -> ()  [unwired: 1 out]
              n588 = Multiply(x=w1089, y=0.25) -> ()  [unwired: 1 out]
              n589 = Increment(x=w1091) -> (x+1=w1094:dbl)
              n590 = Subtract(x=w1079, y=w1090) -> (x-y=w1102:dbl)
              n591 = Subtract(x=w1079, y=w1089) -> (x-y=w1096:dbl)
              n592 = Subtract(x=w1079, y=w1094) -> (x-y=w1093:dbl)
              n593 = Subtract(x=w1079, y=w1091) -> (x-y=w1083:dbl)
              n594 = Add(x=w1079, y=w1091) -> (x+y=w1087:dbl)
              n595 = Add(x=w1079, y=w1089) -> (x+y=w1085:dbl)
              n596 = Add(x=w1079, y=w1090) -> (x+y=w1084:dbl)
              n597 = Add(x=w1079, y=50.0) -> (x+y=w1077:dbl)
              n598 = Add(x=w1083, y=120.0) -> (x+y=w1081:dbl)
              n599 = Add(x=w1077, y=10.0) -> (x+y=w1074:dbl)
              n600 = Increment(x=w1087) -> (x+1=w1086:dbl)
              n601 = Increment(x=w1081) -> (x+1=w1080:dbl)
              n602 = Decrement(x=w1074) -> (x-1=w1075:dbl)
              n603 = Build Array(w1102, w1096, w1093, w1083, w1081, w1080, w1077, w1075, w1074, w1087, w1086, w1085, w1084) -> (w1101:dbl[])
              n604 = for {
                tunnel: w1101 -> [w1106] mode=indexing
                tunnel: dbl[] [-30.0, -30.0, -20.0, 0.0, 0.0, -20.0, -23.0, -20.0, 0.0, 0.0, -20.0, -30.0, -30.0] -> [w1115] mode=indexing
                tunnel: bool[] [FALSE, FALSE, TRUE, TRUE, TRUE, TRUE, TRUE, TRUE, TRUE, TRUE, TRUE, FALSE, FALSE] -> [w1114] mode=indexing
                shift-right: [w1111] -> w1100
                shift-left: w1071 -> [w1113]
                shift-right: [w1107] -> w1067
                shift-left: w1071 -> [w1108]
                tunnel: dbl[] [-30.0, -30.0, -30.0, 0.0, 0.0, -20.0, -23.0, -20.0, 0.0, 0.0, -30.0, -30.0, -30.0] -> [w1105] mode=indexing
                tunnel: bool[] [FALSE, FALSE, FALSE, TRUE, TRUE, TRUE, TRUE, TRUE, TRUE, TRUE, FALSE, FALSE, FALSE] -> [w1104] mode=indexing
                n605 = Bundle By Name(cluster=T3 {"Freq"=0.0, "Limit"=0.0, "dBc Applied?"=FALSE} ("Mask Table"), "Freq"=w1106, "Limit"=w1105, "dBc Applied?"=w1104) -> (w1110:T3)
                n606 = Bundle By Name(cluster=T3 {"Freq"=0.0, "Limit"=0.0, "dBc Applied?"=FALSE} ("Mask Table"), "Freq"=w1106, "Limit"=w1115, "dBc Applied?"=w1114) -> (w1112:T3)
                n607 = Build Array (concatenate)(w1108, w1110) -> (w1107:T1)
                n608 = Build Array (concatenate)(w1113, w1112) -> (w1111:T1)
              }
              n609 = Build Array (concatenate)(w1100, T3 {"Freq"=26500.0, "Limit"=-30.0, "dBc Applied?"=FALSE} ("Mask Table")) -> (w1098:T1)
              n610 = Build Array (concatenate)(w1067, T3 {"Freq"=26500.0, "Limit"=-30.0, "dBc Applied?"=FALSE} ("Mask Table")) -> (w1066:T1)
            }
          }
        }
        frame "Case 2" {
          n611 = case shown="95" w1118 {
            tunnel: [_ w1154 w1205 w1256 w1307 w1358 w1409 w1460 w1511 w1562 w1613] -> w1121
            tunnel: w1120 -> [_ w1153 w1204 w1255 w1306 w1357 w1408 w1459 w1510 w1561 w1612]
            tunnel: w1119 -> [_ w1132 w1186 w1237 w1288 w1337 w1390 w1441 w1492 w1543 w1594]
            tunnel: [_ w1122 w1173 w1224 w1275 w1326 w1377 w1428 w1479 w1530 w1581] -> w1117
            frame 0, Default {
            }
            frame 95 {
              w1127 = T1 [{"Freq"=0.0, "Limit"=-30.0, "dBc Applied?"=FALSE}] ("value")
              n612 = Unbundle By Name(w1153) -> ("BW_N"=w1129:dbl)
              n613 = Multiply(x=1.5, y=w1129) -> (x*y=w1131:dbl)
              n614 = Multiply(x=w1129, y=0.5) -> (x*y=w1134:dbl)
              n615 = Multiply(x=w1129, y=0.25) -> (x*y=w1144:dbl)
              n616 = Multiply(x=w1129, y=0.125) -> ()  [unwired: 1 out]
              n617 = Increment(x=w1134) -> (x+1=w1148:dbl)
              n618 = Subtract(x=w1132, y=w1131) -> (x-y=w1158:dbl)
              n619 = Subtract(x=w1132, y=w1129) -> (x-y=w1152:dbl)
              n620 = Subtract(x=w1132, y=w1148) -> (x-y=w1147:dbl)
              n621 = Subtract(x=w1132, y=w1134) -> (x-y=w1145:dbl)
              n622 = Subtract(x=w1132, y=w1144) -> (x-y=w1143:dbl)
              n623 = Subtract(x=w1132, y=26.55) -> (x-y=w1140:dbl)
              n624 = Subtract(x=w1132, y=0.0) -> (x-y=w1137:dbl)
              n625 = Add(x=w1132, y=w1134) -> (x+y=w1136:dbl)
              n626 = Add(x=w1132, y=w1129) -> (x+y=w1133:dbl)
              n627 = Add(x=w1132, y=w1131) -> (x+y=w1130:dbl)
              n628 = Increment(x=w1143) -> (x+1=w1142:dbl)
              n629 = Decrement(x=w1137) -> (x-1=w1138:dbl)
              n630 = Increment(x=w1136) -> (x+1=w1135:dbl)
              n631 = Build Array(w1158, w1152, w1147, w1145, w1143, w1142, w1140, w1138, w1137, w1136, w1135, w1133, w1130) -> (w1157:dbl[])
              n632 = for {
                tunnel: w1157 -> [w1162] mode=indexing
                tunnel: dbl[] [-30.0, -30.0, -20.0, 0.0, 0.0, -20.0, -23.28, -20.0, 0.0, 0.0, -20.0, -30.0, -30.0] -> [w1171] mode=indexing
                tunnel: bool[] [FALSE, FALSE, TRUE, TRUE, TRUE, TRUE, TRUE, TRUE, TRUE, TRUE, TRUE, FALSE, FALSE] -> [w1170] mode=indexing
                shift-right: [w1167] -> w1156
                shift-left: w1127 -> [w1169]
                shift-right: [w1163] -> w1123
                shift-left: w1127 -> [w1164]
                tunnel: dbl[] [-30.0, -30.0, -30.0, 0.0, 0.0, -20.0, -23.28, -20.0, 0.0, 0.0, -30.0, -30.0, -30.0] -> [w1161] mode=indexing
                tunnel: bool[] [FALSE, FALSE, FALSE, TRUE, TRUE, TRUE, TRUE, TRUE, TRUE, TRUE, FALSE, FALSE, FALSE] -> [w1160] mode=indexing
                n633 = Bundle By Name(cluster=T3 {"Freq"=0.0, "Limit"=0.0, "dBc Applied?"=FALSE} ("Mask Table"), "Freq"=w1162, "Limit"=w1161, "dBc Applied?"=w1160) -> (w1166:T3)
                n634 = Bundle By Name(cluster=T3 {"Freq"=0.0, "Limit"=0.0, "dBc Applied?"=FALSE} ("Mask Table"), "Freq"=w1162, "Limit"=w1171, "dBc Applied?"=w1170) -> (w1168:T3)
                n635 = Build Array (concatenate)(w1164, w1166) -> (w1163:T1)
                n636 = Build Array (concatenate)(w1169, w1168) -> (w1167:T1)
              }
              n637 = Build Array (concatenate)(w1156, T3 {"Freq"=26500.0, "Limit"=-30.0, "dBc Applied?"=FALSE} ("Mask Table")) -> (w1154:T1)
              n638 = Build Array (concatenate)(w1123, T3 {"Freq"=26500.0, "Limit"=-30.0, "dBc Applied?"=FALSE} ("Mask Table")) -> (w1122:T1)
            }
            frame 1094 {
              w1178 = T1 [{"Freq"=0.0, "Limit"=-30.0, "dBc Applied?"=FALSE}] ("value")
              n639 = Unbundle By Name(w1204) -> ("BW_N"=w1183:dbl)
              n640 = Multiply(x=1.5, y=w1183) -> (x*y=w1185:dbl)
              n641 = Multiply(x=w1183, y=0.5) -> (x*y=w1188:dbl)
              n642 = Multiply(x=w1183, y=0.25) -> ()  [unwired: 1 out]
              n643 = Multiply(x=w1183, y=0.125) -> ()  [unwired: 1 out]
              n644 = Increment(x=w1188) -> (x+1=w1201:dbl)
              n645 = Subtract(x=w1186, y=w1185) -> (x-y=w1209:dbl)
              n646 = Subtract(x=w1186, y=w1183) -> (x-y=w1203:dbl)
              n647 = Subtract(x=w1186, y=w1201) -> (x-y=w1200:dbl)
              n648 = Subtract(x=w1186, y=w1188) -> (x-y=w1198:dbl)
              n649 = Subtract(x=w1186, y=0.0) -> (x-y=w1197:dbl)
              n650 = Add(x=w1186, y=26.55) -> (x+y=w1194:dbl)
              n651 = Add(x=w1186, y=40.0) -> (x+y=w1191:dbl)
              n652 = Add(x=w1186, y=w1188) -> (x+y=w1190:dbl)
              n653 = Add(x=w1186, y=w1183) -> (x+y=w1187:dbl)
              n654 = Add(x=w1186, y=w1185) -> (x+y=w1184:dbl)
              n655 = Increment(x=w1197) -> (x+1=w1196:dbl)
              n656 = Decrement(x=w1191) -> (x-1=w1192:dbl)
              n657 = Increment(x=w1190) -> (x+1=w1189:dbl)
              n658 = Build Array(w1209, w1203, w1200, w1198, w1197, w1196, w1194, w1192, w1191, w1190, w1189, w1187, w1184) -> (w1208:dbl[])
              n659 = for {
                tunnel: w1208 -> [w1214] mode=indexing
                tunnel: dbl[] [-30.0, -30.0, -20.0, 0.0, 0.0, -20.0, -23.28, -20.0, 0.0, 0.0, -20.0, -30.0, -30.0] -> [w1222] mode=indexing
                tunnel: bool[] [FALSE, FALSE, TRUE, TRUE, TRUE, TRUE, TRUE, TRUE, TRUE, TRUE, TRUE, FALSE, FALSE] -> [w1221] mode=indexing
                shift-right: [w1218] -> w1207
                shift-left: w1178 -> [w1220]
                shift-right: [w1211] -> w1174
                shift-left: w1178 -> [w1215]
                tunnel: dbl[] [-30.0, -30.0, -30.0, 0.0, 0.0, -20.0, -23.28, -20.0, 0.0, 0.0, -30.0, -30.0, -30.0] -> [w1213] mode=indexing
                tunnel: bool[] [FALSE, FALSE, FALSE, TRUE, TRUE, TRUE, TRUE, TRUE, TRUE, TRUE, FALSE, FALSE, FALSE] -> [w1212] mode=indexing
                n660 = Bundle By Name(cluster=T3 {"Freq"=0.0, "Limit"=0.0, "dBc Applied?"=FALSE} ("Mask Table"), "Freq"=w1214, "Limit"=w1222, "dBc Applied?"=w1221) -> (w1219:T3)
                n661 = Bundle By Name(cluster=T3 {"Freq"=0.0, "Limit"=0.0, "dBc Applied?"=FALSE} ("Mask Table"), "Freq"=w1214, "Limit"=w1213, "dBc Applied?"=w1212) -> (w1217:T3)
                n662 = Build Array (concatenate)(w1220, w1219) -> (w1218:T1)
                n663 = Build Array (concatenate)(w1215, w1217) -> (w1211:T1)
              }
              n664 = Build Array (concatenate)(w1207, T3 {"Freq"=26500.0, "Limit"=-30.0, "dBc Applied?"=FALSE} ("Mask Table")) -> (w1205:T1)
              n665 = Build Array (concatenate)(w1174, T3 {"Freq"=26500.0, "Limit"=-30.0, "dBc Applied?"=FALSE} ("Mask Table")) -> (w1173:T1)
            }
            frame 1104 {
              w1229 = T1 [{"Freq"=0.0, "Limit"=-30.0, "dBc Applied?"=FALSE}] ("value")
              n666 = Unbundle By Name(w1255) -> ("BW_N"=w1234:dbl)
              n667 = Multiply(x=1.5, y=w1234) -> (x*y=w1236:dbl)
              n668 = Multiply(x=w1234, y=0.5) -> (x*y=w1239:dbl)
              n669 = Multiply(x=w1234, y=0.25) -> ()  [unwired: 1 out]
              n670 = Multiply(x=w1234, y=0.125) -> ()  [unwired: 1 out]
              n671 = Increment(x=w1239) -> (x+1=w1252:dbl)
              n672 = Subtract(x=w1237, y=w1236) -> (x-y=w1260:dbl)
              n673 = Subtract(x=w1237, y=w1234) -> (x-y=w1254:dbl)
              n674 = Subtract(x=w1237, y=w1252) -> (x-y=w1251:dbl)
              n675 = Subtract(x=w1237, y=w1239) -> (x-y=w1249:dbl)
              n676 = Subtract(x=w1237, y=80.0) -> (x-y=w1248:dbl)
              n677 = Subtract(x=w1237, y=53.22) -> (x-y=w1245:dbl)
              n678 = Add(x=w1237, y=0.0) -> (x+y=w1242:dbl)
              n679 = Add(x=w1237, y=w1239) -> (x+y=w1241:dbl)
              n680 = Add(x=w1237, y=w1234) -> (x+y=w1238:dbl)
              n681 = Add(x=w1237, y=w1236) -> (x+y=w1235:dbl)
              n682 = Increment(x=w1248) -> (x+1=w1247:dbl)
              n683 = Decrement(x=w1242) -> (x-1=w1243:dbl)
              n684 = Increment(x=w1241) -> (x+1=w1240:dbl)
              n685 = Build Array(w1260, w1254, w1251, w1249, w1248, w1247, w1245, w1243, w1242, w1241, w1240, w1238, w1235) -> (w1259:dbl[])
              n686 = for {
                tunnel: w1259 -> [w1264] mode=indexing
                tunnel: dbl[] [-30.0, -30.0, -20.0, 0.0, 0.0, -20.0, -23.31, -20.0, 0.0, 0.0, -20.0, -30.0, -30.0] -> [w1273] mode=indexing
                tunnel: bool[] [FALSE, FALSE, TRUE, TRUE, TRUE, TRUE, TRUE, TRUE, TRUE, TRUE, TRUE, FALSE, FALSE] -> [w1272] mode=indexing
                shift-right: [w1269] -> w1258
                shift-left: w1229 -> [w1271]
                shift-right: [w1265] -> w1225
                shift-left: w1229 -> [w1266]
                tunnel: dbl[] [-30.0, -30.0, -30.0, 0.0, 0.0, -20.0, -23.31, -20.0, 0.0, 0.0, -30.0, -30.0, -30.0] -> [w1263] mode=indexing
                tunnel: bool[] [FALSE, FALSE, FALSE, TRUE, TRUE, TRUE, TRUE, TRUE, TRUE, TRUE, FALSE, FALSE, FALSE] -> [w1262] mode=indexing
                n687 = Bundle By Name(cluster=T3 {"Freq"=0.0, "Limit"=0.0, "dBc Applied?"=FALSE} ("Mask Table"), "Freq"=w1264, "Limit"=w1263, "dBc Applied?"=w1262) -> (w1268:T3)
                n688 = Bundle By Name(cluster=T3 {"Freq"=0.0, "Limit"=0.0, "dBc Applied?"=FALSE} ("Mask Table"), "Freq"=w1264, "Limit"=w1273, "dBc Applied?"=w1272) -> (w1270:T3)
                n689 = Build Array (concatenate)(w1266, w1268) -> (w1265:T1)
                n690 = Build Array (concatenate)(w1271, w1270) -> (w1269:T1)
              }
              n691 = Build Array (concatenate)(w1225, T3 {"Freq"=26500.0, "Limit"=-30.0, "dBc Applied?"=FALSE} ("Mask Table")) -> (w1224:T1)
              n692 = Build Array (concatenate)(w1258, T3 {"Freq"=26500.0, "Limit"=-30.0, "dBc Applied?"=FALSE} ("Mask Table")) -> (w1256:T1)
            }
            frame 10104 {
              w1280 = T1 [{"Freq"=0.0, "Limit"=-30.0, "dBc Applied?"=FALSE}] ("value")
              n693 = Unbundle By Name(w1306) -> ("BW_N"=w1285:dbl)
              n694 = Multiply(x=1.5, y=w1285) -> (x*y=w1287:dbl)
              n695 = Multiply(x=w1285, y=0.5) -> (x*y=w1290:dbl)
              n696 = Multiply(x=w1285, y=0.25) -> ()  [unwired: 1 out]
              n697 = Multiply(x=w1285, y=0.125) -> ()  [unwired: 1 out]
              n698 = Increment(x=w1290) -> (x+1=w1303:dbl)
              n699 = Subtract(x=w1288, y=w1287) -> (x-y=w1311:dbl)
              n700 = Subtract(x=w1288, y=w1285) -> (x-y=w1305:dbl)
              n701 = Subtract(x=w1288, y=w1303) -> (x-y=w1302:dbl)
              n702 = Subtract(x=w1288, y=w1290) -> (x-y=w1300:dbl)
              n703 = Subtract(x=w1288, y=0.0) -> (x-y=w1299:dbl)
              n704 = Subtract(x=w1288, y=-53.22) -> (x-y=w1296:dbl)
              n705 = Add(x=w1288, y=80.0) -> (x+y=w1293:dbl)
              n706 = Add(x=w1288, y=w1290) -> (x+y=w1292:dbl)
              n707 = Add(x=w1288, y=w1285) -> (x+y=w1289:dbl)
              n708 = Add(x=w1288, y=w1287) -> (x+y=w1286:dbl)
              n709 = Increment(x=w1299) -> (x+1=w1298:dbl)
              n710 = Decrement(x=w1293) -> (x-1=w1294:dbl)
              n711 = Increment(x=w1292) -> (x+1=w1291:dbl)
              n712 = Build Array(w1311, w1305, w1302, w1300, w1299, w1298, w1296, w1294, w1293, w1292, w1291, w1289, w1286) -> (w1310:dbl[])
              n713 = for {
                tunnel: w1310 -> [w1315] mode=indexing
                tunnel: dbl[] [-30.0, -30.0, -20.0, 0.0, 0.0, -20.0, -23.31, -20.0, 0.0, 0.0, -20.0, -30.0, -30.0] -> [w1324] mode=indexing
                tunnel: bool[] [FALSE, FALSE, TRUE, TRUE, TRUE, TRUE, TRUE, TRUE, TRUE, TRUE, TRUE, FALSE, FALSE] -> [w1323] mode=indexing
                shift-right: [w1320] -> w1309
                shift-left: w1280 -> [w1322]
                shift-right: [w1316] -> w1276
                shift-left: w1280 -> [w1317]
                tunnel: dbl[] [-30.0, -30.0, -30.0, 0.0, 0.0, -20.0, -23.31, -20.0, 0.0, 0.0, -30.0, -30.0, -30.0] -> [w1314] mode=indexing
                tunnel: bool[] [FALSE, FALSE, FALSE, TRUE, TRUE, TRUE, TRUE, TRUE, TRUE, TRUE, FALSE, FALSE, FALSE] -> [w1313] mode=indexing
                n714 = Bundle By Name(cluster=T3 {"Freq"=0.0, "Limit"=0.0, "dBc Applied?"=FALSE} ("Mask Table"), "Freq"=w1315, "Limit"=w1314, "dBc Applied?"=w1313) -> (w1319:T3)
                n715 = Bundle By Name(cluster=T3 {"Freq"=0.0, "Limit"=0.0, "dBc Applied?"=FALSE} ("Mask Table"), "Freq"=w1315, "Limit"=w1324, "dBc Applied?"=w1323) -> (w1321:T3)
                n716 = Build Array (concatenate)(w1317, w1319) -> (w1316:T1)
                n717 = Build Array (concatenate)(w1322, w1321) -> (w1320:T1)
              }
              n718 = Build Array (concatenate)(w1309, T3 {"Freq"=26500.0, "Limit"=-30.0, "dBc Applied?"=FALSE} ("Mask Table")) -> (w1307:T1)
              n719 = Build Array (concatenate)(w1276, T3 {"Freq"=26500.0, "Limit"=-30.0, "dBc Applied?"=FALSE} ("Mask Table")) -> (w1275:T1)
            }
            frame 106 {
              w1331 = T1 [{"Freq"=0.0, "Limit"=-30.0, "dBc Applied?"=FALSE}] ("value")
              n720 = Unbundle By Name(w1357) -> ("BW_N"=w1334:dbl)
              n721 = Multiply(x=1.5, y=w1334) -> (x*y=w1336:dbl)
              n722 = Multiply(x=w1334, y=0.5) -> (x*y=w1339:dbl)
              n723 = Multiply(x=w1334, y=0.25) -> ()  [unwired: 1 out]
              n724 = Multiply(x=w1334, y=0.125) -> ()  [unwired: 1 out]
              n725 = Increment(x=w1339) -> (x+1=w1352:dbl)
              n726 = Subtract(x=w1337, y=w1336) -> (x-y=w1362:dbl)
              n727 = Subtract(x=w1337, y=w1334) -> (x-y=w1356:dbl)
              n728 = Subtract(x=w1337, y=w1352) -> (x-y=w1351:dbl)
              n729 = Subtract(x=w1337, y=w1339) -> (x-y=w1349:dbl)
              n730 = Subtract(x=w1337, y=120.0) -> (x-y=w1348:dbl)
              n731 = Subtract(x=w1337, y=113.77) -> (x-y=w1345:dbl)
              n732 = Add(x=w1337, y=-80.0) -> (x+y=w1342:dbl)
              n733 = Add(x=w1337, y=w1339) -> (x+y=w1341:dbl)
              n734 = Add(x=w1337, y=w1334) -> (x+y=w1338:dbl)
              n735 = Add(x=w1337, y=w1336) -> (x+y=w1335:dbl)
              n736 = Increment(x=w1348) -> (x+1=w1347:dbl)
              n737 = Decrement(x=w1342) -> (x-1=w1343:dbl)
              n738 = Increment(x=w1341) -> (x+1=w1340:dbl)
              n739 = Build Array(w1362, w1356, w1351, w1349, w1348, w1347, w1345, w1343, w1342, w1341, w1340, w1338, w1335) -> (w1361:dbl[])
              n740 = for {
                tunnel: w1361 -> [w1366] mode=indexing
                tunnel: dbl[] [-30.0, -30.0, -20.0, 0.0, 0.0, -20.0, -21.38, -20.0, 0.0, 0.0, -20.0, -30.0, -30.0] -> [w1375] mode=indexing
                tunnel: bool[] [FALSE, FALSE, TRUE, TRUE, TRUE, TRUE, TRUE, TRUE, TRUE, TRUE, TRUE, FALSE, FALSE] -> [w1374] mode=indexing
                shift-right: [w1371] -> w1360
                shift-left: w1331 -> [w1373]
                shift-right: [w1367] -> w1327
                shift-left: w1331 -> [w1368]
                tunnel: dbl[] [-30.0, -30.0, -30.0, 0.0, 0.0, -20.0, -21.38, -20.0, 0.0, 0.0, -30.0, -30.0, -30.0] -> [w1365] mode=indexing
                tunnel: bool[] [FALSE, FALSE, FALSE, TRUE, TRUE, TRUE, TRUE, TRUE, TRUE, TRUE, FALSE, FALSE, FALSE] -> [w1364] mode=indexing
                n741 = Bundle By Name(cluster=T3 {"Freq"=0.0, "Limit"=0.0, "dBc Applied?"=FALSE} ("Mask Table"), "Freq"=w1366, "Limit"=w1365, "dBc Applied?"=w1364) -> (w1370:T3)
                n742 = Bundle By Name(cluster=T3 {"Freq"=0.0, "Limit"=0.0, "dBc Applied?"=FALSE} ("Mask Table"), "Freq"=w1366, "Limit"=w1375, "dBc Applied?"=w1374) -> (w1372:T3)
                n743 = Build Array (concatenate)(w1368, w1370) -> (w1367:T1)
                n744 = Build Array (concatenate)(w1373, w1372) -> (w1371:T1)
              }
              n745 = Build Array (concatenate)(w1327, T3 {"Freq"=26500.0, "Limit"=-30.0, "dBc Applied?"=FALSE} ("Mask Table")) -> (w1326:T1)
              n746 = Build Array (concatenate)(w1360, T3 {"Freq"=26500.0, "Limit"=-30.0, "dBc Applied?"=FALSE} ("Mask Table")) -> (w1358:T1)
            }
            frame 1105 {
              w1382 = T1 [{"Freq"=0.0, "Limit"=-30.0, "dBc Applied?"=FALSE}] ("value")
              n747 = Unbundle By Name(w1408) -> ("BW_N"=w1387:dbl)
              n748 = Multiply(x=1.5, y=w1387) -> (x*y=w1389:dbl)
              n749 = Multiply(x=w1387, y=0.5) -> (x*y=w1392:dbl)
              n750 = Multiply(x=w1387, y=0.25) -> ()  [unwired: 1 out]
              n751 = Multiply(x=w1387, y=0.125) -> ()  [unwired: 1 out]
              n752 = Increment(x=w1392) -> (x+1=w1405:dbl)
              n753 = Subtract(x=w1390, y=w1389) -> (x-y=w1413:dbl)
              n754 = Subtract(x=w1390, y=w1387) -> (x-y=w1407:dbl)
              n755 = Subtract(x=w1390, y=w1405) -> (x-y=w1404:dbl)
              n756 = Subtract(x=w1390, y=w1392) -> (x-y=w1402:dbl)
              n757 = Subtract(x=w1390, y=80.0) -> (x-y=w1401:dbl)
              n758 = Subtract(x=w1390, y=68.26) -> (x-y=w1398:dbl)
              n759 = Add(x=w1390, y=-40.0) -> (x+y=w1395:dbl)
              n760 = Add(x=w1390, y=w1392) -> (x+y=w1394:dbl)
              n761 = Add(x=w1390, y=w1387) -> (x+y=w1391:dbl)
              n762 = Add(x=w1390, y=w1389) -> (x+y=w1388:dbl)
              n763 = Increment(x=w1401) -> (x+1=w1400:dbl)
              n764 = Decrement(x=w1395) -> (x-1=w1396:dbl)
              n765 = Increment(x=w1394) -> (x+1=w1393:dbl)
              n766 = Build Array(w1413, w1407, w1404, w1402, w1401, w1400, w1398, w1396, w1395, w1394, w1393, w1391, w1388) -> (w1412:dbl[])
              n767 = for {
                tunnel: w1412 -> [w1417] mode=indexing
                tunnel: dbl[] [-30.0, -30.0, -20.0, 0.0, 0.0, -20.0, -21.38, -20.0, 0.0, 0.0, -20.0, -30.0, -30.0] -> [w1426] mode=indexing
                tunnel: bool[] [FALSE, FALSE, TRUE, TRUE, TRUE, TRUE, TRUE, TRUE, TRUE, TRUE, TRUE, FALSE, FALSE] -> [w1425] mode=indexing
                shift-right: [w1422] -> w1411
                shift-left: w1382 -> [w1424]
                shift-right: [w1418] -> w1378
                shift-left: w1382 -> [w1419]
                tunnel: dbl[] [-30.0, -30.0, -30.0, 0.0, 0.0, -20.0, -21.38, -20.0, 0.0, 0.0, -30.0, -30.0, -30.0] -> [w1416] mode=indexing
                tunnel: bool[] [FALSE, FALSE, FALSE, TRUE, TRUE, TRUE, TRUE, TRUE, TRUE, TRUE, FALSE, FALSE, FALSE] -> [w1415] mode=indexing
                n768 = Bundle By Name(cluster=T3 {"Freq"=0.0, "Limit"=0.0, "dBc Applied?"=FALSE} ("Mask Table"), "Freq"=w1417, "Limit"=w1426, "dBc Applied?"=w1425) -> (w1423:T3)
                n769 = Bundle By Name(cluster=T3 {"Freq"=0.0, "Limit"=0.0, "dBc Applied?"=FALSE} ("Mask Table"), "Freq"=w1417, "Limit"=w1416, "dBc Applied?"=w1415) -> (w1421:T3)
                n770 = Build Array (concatenate)(w1424, w1423) -> (w1422:T1)
                n771 = Build Array (concatenate)(w1419, w1421) -> (w1418:T1)
              }
              n772 = Build Array (concatenate)(w1378, T3 {"Freq"=26500.0, "Limit"=-30.0, "dBc Applied?"=FALSE} ("Mask Table")) -> (w1377:T1)
              n773 = Build Array (concatenate)(w1411, T3 {"Freq"=26500.0, "Limit"=-30.0, "dBc Applied?"=FALSE} ("Mask Table")) -> (w1409:T1)
            }
            frame 1106 {
              w1433 = T1 [{"Freq"=0.0, "Limit"=-30.0, "dBc Applied?"=FALSE}] ("value")
              n774 = Unbundle By Name(w1459) -> ("BW_N"=w1438:dbl)
              n775 = Multiply(x=1.5, y=w1438) -> (x*y=w1440:dbl)
              n776 = Multiply(x=w1438, y=0.5) -> (x*y=w1443:dbl)
              n777 = Multiply(x=w1438, y=0.25) -> ()  [unwired: 1 out]
              n778 = Multiply(x=w1438, y=0.125) -> ()  [unwired: 1 out]
              n779 = Increment(x=w1443) -> (x+1=w1456:dbl)
              n780 = Subtract(x=w1441, y=w1440) -> (x-y=w1464:dbl)
              n781 = Subtract(x=w1441, y=w1438) -> (x-y=w1458:dbl)
              n782 = Subtract(x=w1441, y=w1456) -> (x-y=w1455:dbl)
              n783 = Subtract(x=w1441, y=w1443) -> (x-y=w1453:dbl)
              n784 = Subtract(x=w1441, y=40.0) -> (x-y=w1452:dbl)
              n785 = Subtract(x=w1441, y=22.75) -> (x-y=w1449:dbl)
              n786 = Add(x=w1441, y=0.0) -> (x+y=w1446:dbl)
              n787 = Add(x=w1441, y=w1443) -> (x+y=w1445:dbl)
              n788 = Add(x=w1441, y=w1438) -> (x+y=w1442:dbl)
              n789 = Add(x=w1441, y=w1440) -> (x+y=w1439:dbl)
              n790 = Increment(x=w1452) -> (x+1=w1451:dbl)
              n791 = Decrement(x=w1446) -> (x-1=w1447:dbl)
              n792 = Increment(x=w1445) -> (x+1=w1444:dbl)
              n793 = Build Array(w1464, w1458, w1455, w1453, w1452, w1451, w1449, w1447, w1446, w1445, w1444, w1442, w1439) -> (w1463:dbl[])
              n794 = for {
                tunnel: w1463 -> [w1468] mode=indexing
                tunnel: dbl[] [-30.0, -30.0, -20.0, 0.0, 0.0, -20.0, -21.38, -20.0, 0.0, 0.0, -20.0, -30.0, -30.0] -> [w1477] mode=indexing
                tunnel: bool[] [FALSE, FALSE, TRUE, TRUE, TRUE, TRUE, TRUE, TRUE, TRUE, TRUE, TRUE, FALSE, FALSE] -> [w1476] mode=indexing
                shift-right: [w1473] -> w1462
                shift-left: w1433 -> [w1475]
                shift-right: [w1469] -> w1429
                shift-left: w1433 -> [w1470]
                tunnel: dbl[] [-30.0, -30.0, -30.0, 0.0, 0.0, -20.0, -21.38, -20.0, 0.0, 0.0, -30.0, -30.0, -30.0] -> [w1467] mode=indexing
                tunnel: bool[] [FALSE, FALSE, FALSE, TRUE, TRUE, TRUE, TRUE, TRUE, TRUE, TRUE, FALSE, FALSE, FALSE] -> [w1466] mode=indexing
                n795 = Bundle By Name(cluster=T3 {"Freq"=0.0, "Limit"=0.0, "dBc Applied?"=FALSE} ("Mask Table"), "Freq"=w1468, "Limit"=w1477, "dBc Applied?"=w1476) -> (w1474:T3)
                n796 = Bundle By Name(cluster=T3 {"Freq"=0.0, "Limit"=0.0, "dBc Applied?"=FALSE} ("Mask Table"), "Freq"=w1468, "Limit"=w1467, "dBc Applied?"=w1466) -> (w1472:T3)
                n797 = Build Array (concatenate)(w1475, w1474) -> (w1473:T1)
                n798 = Build Array (concatenate)(w1470, w1472) -> (w1469:T1)
              }
              n799 = Build Array (concatenate)(w1462, T3 {"Freq"=26500.0, "Limit"=-30.0, "dBc Applied?"=FALSE} ("Mask Table")) -> (w1460:T1)
              n800 = Build Array (concatenate)(w1429, T3 {"Freq"=26500.0, "Limit"=-30.0, "dBc Applied?"=FALSE} ("Mask Table")) -> (w1428:T1)
            }
            frame 10105 {
              w1484 = T1 [{"Freq"=0.0, "Limit"=-30.0, "dBc Applied?"=FALSE}] ("value")
              n801 = Unbundle By Name(w1510) -> ("BW_N"=w1489:dbl)
              n802 = Multiply(x=1.5, y=w1489) -> (x*y=w1491:dbl)
              n803 = Multiply(x=w1489, y=0.5) -> (x*y=w1494:dbl)
              n804 = Multiply(x=w1489, y=0.25) -> ()  [unwired: 1 out]
              n805 = Multiply(x=w1489, y=0.125) -> ()  [unwired: 1 out]
              n806 = Increment(x=w1494) -> (x+1=w1507:dbl)
              n807 = Subtract(x=w1492, y=w1491) -> (x-y=w1515:dbl)
              n808 = Subtract(x=w1492, y=w1489) -> (x-y=w1509:dbl)
              n809 = Subtract(x=w1492, y=w1507) -> (x-y=w1506:dbl)
              n810 = Subtract(x=w1492, y=w1494) -> (x-y=w1504:dbl)
              n811 = Subtract(x=w1492, y=0.0) -> (x-y=w1503:dbl)
              n812 = Subtract(x=w1492, y=-22.75) -> (x-y=w1500:dbl)
              n813 = Add(x=w1492, y=40.0) -> (x+y=w1497:dbl)
              n814 = Add(x=w1492, y=w1494) -> (x+y=w1496:dbl)
              n815 = Add(x=w1492, y=w1489) -> (x+y=w1493:dbl)
              n816 = Add(x=w1492, y=w1491) -> (x+y=w1490:dbl)
              n817 = Increment(x=w1503) -> (x+1=w1502:dbl)
              n818 = Decrement(x=w1497) -> (x-1=w1498:dbl)
              n819 = Increment(x=w1496) -> (x+1=w1495:dbl)
              n820 = Build Array(w1515, w1509, w1506, w1504, w1503, w1502, w1500, w1498, w1497, w1496, w1495, w1493, w1490) -> (w1514:dbl[])
              n821 = for {
                tunnel: w1514 -> [w1519] mode=indexing
                tunnel: dbl[] [-30.0, -30.0, -20.0, 0.0, 0.0, -20.0, -21.38, -20.0, 0.0, 0.0, -20.0, -30.0, -30.0] -> [w1528] mode=indexing
                tunnel: bool[] [FALSE, FALSE, TRUE, TRUE, TRUE, TRUE, TRUE, TRUE, TRUE, TRUE, TRUE, FALSE, FALSE] -> [w1527] mode=indexing
                shift-right: [w1524] -> w1513
                shift-left: w1484 -> [w1526]
                shift-right: [w1520] -> w1480
                shift-left: w1484 -> [w1521]
                tunnel: dbl[] [-30.0, -30.0, -30.0, 0.0, 0.0, -20.0, -21.38, -20.0, 0.0, 0.0, -30.0, -30.0, -30.0] -> [w1518] mode=indexing
                tunnel: bool[] [FALSE, FALSE, FALSE, TRUE, TRUE, TRUE, TRUE, TRUE, TRUE, TRUE, FALSE, FALSE, FALSE] -> [w1517] mode=indexing
                n822 = Bundle By Name(cluster=T3 {"Freq"=0.0, "Limit"=0.0, "dBc Applied?"=FALSE} ("Mask Table"), "Freq"=w1519, "Limit"=w1528, "dBc Applied?"=w1527) -> (w1525:T3)
                n823 = Bundle By Name(cluster=T3 {"Freq"=0.0, "Limit"=0.0, "dBc Applied?"=FALSE} ("Mask Table"), "Freq"=w1519, "Limit"=w1518, "dBc Applied?"=w1517) -> (w1523:T3)
                n824 = Build Array (concatenate)(w1526, w1525) -> (w1524:T1)
                n825 = Build Array (concatenate)(w1521, w1523) -> (w1520:T1)
              }
              n826 = Build Array (concatenate)(w1513, T3 {"Freq"=26500.0, "Limit"=-30.0, "dBc Applied?"=FALSE} ("Mask Table")) -> (w1511:T1)
              n827 = Build Array (concatenate)(w1480, T3 {"Freq"=26500.0, "Limit"=-30.0, "dBc Applied?"=FALSE} ("Mask Table")) -> (w1479:T1)
            }
            frame 10106 {
              w1535 = T1 [{"Freq"=0.0, "Limit"=-30.0, "dBc Applied?"=FALSE}] ("value")
              n828 = Unbundle By Name(w1561) -> ("BW_N"=w1540:dbl)
              n829 = Multiply(x=1.5, y=w1540) -> (x*y=w1542:dbl)
              n830 = Multiply(x=w1540, y=0.5) -> (x*y=w1545:dbl)
              n831 = Multiply(x=w1540, y=0.25) -> ()  [unwired: 1 out]
              n832 = Multiply(x=w1540, y=0.125) -> ()  [unwired: 1 out]
              n833 = Increment(x=w1545) -> (x+1=w1558:dbl)
              n834 = Subtract(x=w1543, y=w1542) -> (x-y=w1566:dbl)
              n835 = Subtract(x=w1543, y=w1540) -> (x-y=w1560:dbl)
              n836 = Subtract(x=w1543, y=w1558) -> (x-y=w1557:dbl)
              n837 = Subtract(x=w1543, y=w1545) -> (x-y=w1555:dbl)
              n838 = Add(x=w1543, y=40.0) -> (x+y=w1554:dbl)
              n839 = Subtract(x=w1543, y=-68.26) -> (x-y=w1551:dbl)
              n840 = Add(x=w1543, y=80.0) -> (x+y=w1548:dbl)
              n841 = Add(x=w1543, y=w1545) -> (x+y=w1547:dbl)
              n842 = Add(x=w1543, y=w1540) -> (x+y=w1544:dbl)
              n843 = Add(x=w1543, y=w1542) -> (x+y=w1541:dbl)
              n844 = Increment(x=w1554) -> (x+1=w1553:dbl)
              n845 = Decrement(x=w1548) -> (x-1=w1549:dbl)
              n846 = Increment(x=w1547) -> (x+1=w1546:dbl)
              n847 = Build Array(w1566, w1560, w1557, w1555, w1554, w1553, w1551, w1549, w1548, w1547, w1546, w1544, w1541) -> (w1565:dbl[])
              n848 = for {
                tunnel: w1565 -> [w1570] mode=indexing
                tunnel: dbl[] [-30.0, -30.0, -20.0, 0.0, 0.0, -20.0, -21.38, -20.0, 0.0, 0.0, -20.0, -30.0, -30.0] -> [w1579] mode=indexing
                tunnel: bool[] [FALSE, FALSE, TRUE, TRUE, TRUE, TRUE, TRUE, TRUE, TRUE, TRUE, TRUE, FALSE, FALSE] -> [w1578] mode=indexing
                shift-right: [w1575] -> w1564
                shift-left: w1535 -> [w1577]
                shift-right: [w1571] -> w1531
                shift-left: w1535 -> [w1572]
                tunnel: dbl[] [-30.0, -30.0, -30.0, 0.0, 0.0, -20.0, -21.38, -20.0, 0.0, 0.0, -30.0, -30.0, -30.0] -> [w1569] mode=indexing
                tunnel: bool[] [FALSE, FALSE, FALSE, TRUE, TRUE, TRUE, TRUE, TRUE, TRUE, TRUE, FALSE, FALSE, FALSE] -> [w1568] mode=indexing
                n849 = Bundle By Name(cluster=T3 {"Freq"=0.0, "Limit"=0.0, "dBc Applied?"=FALSE} ("Mask Table"), "Freq"=w1570, "Limit"=w1569, "dBc Applied?"=w1568) -> (w1574:T3)
                n850 = Bundle By Name(cluster=T3 {"Freq"=0.0, "Limit"=0.0, "dBc Applied?"=FALSE} ("Mask Table"), "Freq"=w1570, "Limit"=w1579, "dBc Applied?"=w1578) -> (w1576:T3)
                n851 = Build Array (concatenate)(w1572, w1574) -> (w1571:T1)
                n852 = Build Array (concatenate)(w1577, w1576) -> (w1575:T1)
              }
              n853 = Build Array (concatenate)(w1564, T3 {"Freq"=26500.0, "Limit"=-30.0, "dBc Applied?"=FALSE} ("Mask Table")) -> (w1562:T1)
              n854 = Build Array (concatenate)(w1531, T3 {"Freq"=26500.0, "Limit"=-30.0, "dBc Applied?"=FALSE} ("Mask Table")) -> (w1530:T1)
            }
            frame 11105 {
              w1586 = T1 [{"Freq"=0.0, "Limit"=-30.0, "dBc Applied?"=FALSE}] ("value")
              n855 = Unbundle By Name(w1612) -> ("BW_N"=w1591:dbl)
              n856 = Multiply(x=1.5, y=w1591) -> (x*y=w1593:dbl)
              n857 = Multiply(x=w1591, y=0.5) -> (x*y=w1596:dbl)
              n858 = Multiply(x=w1591, y=0.25) -> ()  [unwired: 1 out]
              n859 = Multiply(x=w1591, y=0.125) -> ()  [unwired: 1 out]
              n860 = Increment(x=w1596) -> (x+1=w1609:dbl)
              n861 = Subtract(x=w1594, y=w1593) -> (x-y=w1617:dbl)
              n862 = Subtract(x=w1594, y=w1591) -> (x-y=w1611:dbl)
              n863 = Subtract(x=w1594, y=w1609) -> (x-y=w1608:dbl)
              n864 = Subtract(x=w1594, y=w1596) -> (x-y=w1606:dbl)
              n865 = Add(x=w1594, y=80.0) -> (x+y=w1605:dbl)
              n866 = Subtract(x=w1594, y=-113.77) -> (x-y=w1602:dbl)
              n867 = Add(x=w1594, y=120.0) -> (x+y=w1599:dbl)
              n868 = Add(x=w1594, y=w1596) -> (x+y=w1598:dbl)
              n869 = Add(x=w1594, y=w1591) -> (x+y=w1595:dbl)
              n870 = Add(x=w1594, y=w1593) -> (x+y=w1592:dbl)
              n871 = Increment(x=w1605) -> (x+1=w1604:dbl)
              n872 = Decrement(x=w1599) -> (x-1=w1600:dbl)
              n873 = Increment(x=w1598) -> (x+1=w1597:dbl)
              n874 = Build Array(w1617, w1611, w1608, w1606, w1605, w1604, w1602, w1600, w1599, w1598, w1597, w1595, w1592) -> (w1616:dbl[])
              n875 = for {
                tunnel: w1616 -> [w1621] mode=indexing
                tunnel: dbl[] [-30.0, -30.0, -20.0, 0.0, 0.0, -20.0, -21.38, -20.0, 0.0, 0.0, -20.0, -30.0, -30.0] -> [w1630] mode=indexing
                tunnel: bool[] [FALSE, FALSE, TRUE, TRUE, TRUE, TRUE, TRUE, TRUE, TRUE, TRUE, TRUE, FALSE, FALSE] -> [w1629] mode=indexing
                shift-right: [w1626] -> w1615
                shift-left: w1586 -> [w1628]
                shift-right: [w1622] -> w1582
                shift-left: w1586 -> [w1623]
                tunnel: dbl[] [-30.0, -30.0, -30.0, 0.0, 0.0, -20.0, -21.38, -20.0, 0.0, 0.0, -30.0, -30.0, -30.0] -> [w1620] mode=indexing
                tunnel: bool[] [FALSE, FALSE, FALSE, TRUE, TRUE, TRUE, TRUE, TRUE, TRUE, TRUE, FALSE, FALSE, FALSE] -> [w1619] mode=indexing
                n876 = Bundle By Name(cluster=T3 {"Freq"=0.0, "Limit"=0.0, "dBc Applied?"=FALSE} ("Mask Table"), "Freq"=w1621, "Limit"=w1630, "dBc Applied?"=w1629) -> (w1627:T3)
                n877 = Bundle By Name(cluster=T3 {"Freq"=0.0, "Limit"=0.0, "dBc Applied?"=FALSE} ("Mask Table"), "Freq"=w1621, "Limit"=w1620, "dBc Applied?"=w1619) -> (w1625:T3)
                n878 = Build Array (concatenate)(w1628, w1627) -> (w1626:T1)
                n879 = Build Array (concatenate)(w1623, w1625) -> (w1622:T1)
              }
              n880 = Build Array (concatenate)(w1615, T3 {"Freq"=26500.0, "Limit"=-30.0, "dBc Applied?"=FALSE} ("Mask Table")) -> (w1613:T1)
              n881 = Build Array (concatenate)(w1582, T3 {"Freq"=26500.0, "Limit"=-30.0, "dBc Applied?"=FALSE} ("Mask Table")) -> (w1581:T1)
            }
          }
        }
        frame "Case 1+2" {
          n882 = case shown="11102" w1633 {
            tunnel: [_ w1669 w1721 w1773 w1825 w1877 w1929 w1981 w2033] -> w1636
            tunnel: w1635 -> [_ w1668 w1720 w1772 w1824 w1876 w1928 w1980 w2032]
            tunnel: w1634 -> [_ w1646 w1699 w1751 w1803 w1855 w1907 w1959 w2011]
            tunnel: [_ w1637 w1688 w1740 w1792 w1844 w1896 w1948 w2000] -> w1632
            frame 0, Default {
            }
            frame 101 {
              w1653 = 80.0 ("y")
              w1642 = T1 [{"Freq"=0.0, "Limit"=-30.0, "dBc Applied?"=FALSE}] ("value")
              n883 = Unbundle By Name(w1668) -> ("BW_N"=w1648:dbl)
              n884 = Multiply(x=1.5, y=w1648) -> (x*y=w1645:dbl)
              n885 = Subtract(x=w1646, y=w1645) -> (x-y=w1673:dbl)
              n886 = Subtract(x=w1646, y=w1648) -> (x-y=w1667:dbl)
              n887 = Subtract(x=w1646, y=280.0) -> (x-y=w1665:dbl)
              n888 = Subtract(x=w1646, y=160.0) -> (x-y=w1661:dbl)
              n889 = Subtract(x=w1646, y=w1653) -> (x-y=w1655:dbl)
              n890 = Subtract(x=w1646, y=120.0) -> (x-y=w1659:dbl)
              n891 = Subtract(x=w1646, y=111.63) -> (x-y=w1656:dbl)
              n892 = Add(x=w1646, y=w1653) -> (x+y=w1652:dbl)
              n893 = Add(x=w1646, y=200.0) -> (x+y=w1649:dbl)
              n894 = Add(x=w1646, y=w1648) -> (x+y=w1647:dbl)
              n895 = Add(x=w1646, y=w1645) -> (x+y=w1644:dbl)
              n896 = Decrement(x=w1661) -> (x-1=w1662:dbl)
              n897 = Increment(x=w1659) -> (x+1=w1658:dbl)
              n898 = Increment(x=w1652) -> (x+1=w1651:dbl)
              n899 = Decrement(x=w1655) -> (x-1=w1654:dbl)
              n900 = Build Array(w1673, w1667, w1665, w1662, w1661, w1659, w1658, w1656, w1654, w1655, w1652, w1651, w1649, w1647, w1644) -> (w1672:dbl[])
              n901 = for {
                tunnel: w1672 -> [w1677] mode=indexing
                tunnel: dbl[] [-30.0, -30.0, -30.0, -20.0, 0.0, 0.0, -20.0, -21.94, -20.0, 0.0, 0.0, -20.0, -30.0, -30.0, -30.0] -> [w1686] mode=indexing
                tunnel: bool[] [FALSE, FALSE, FALSE, TRUE, TRUE, TRUE, TRUE, TRUE, TRUE, TRUE, TRUE, TRUE, FALSE, FALSE, FALSE] -> [w1685] mode=indexing
                shift-right: [w1682] -> w1671
                shift-left: w1642 -> [w1684]
                shift-right: [w1678] -> w1638
                shift-left: w1642 -> [w1679]
                tunnel: dbl[] [-30.0, -30.0, -30.0, -30.0, 0.0, 0.0, -20.0, -21.94, -20.0, 0.0, 0.0, -30.0, -30.0, -30.0, -30.0] -> [w1676] mode=indexing
                tunnel: bool[] [FALSE, FALSE, FALSE, FALSE, TRUE, TRUE, TRUE, TRUE, TRUE, TRUE, TRUE, FALSE, FALSE, FALSE, FALSE] -> [w1675] mode=indexing
                n902 = Bundle By Name(cluster=T3 {"Freq"=0.0, "Limit"=0.0, "dBc Applied?"=FALSE} ("Mask Table"), "Freq"=w1677, "Limit"=w1686, "dBc Applied?"=w1685) -> (w1683:T3)
                n903 = Bundle By Name(cluster=T3 {"Freq"=0.0, "Limit"=0.0, "dBc Applied?"=FALSE} ("Mask Table"), "Freq"=w1677, "Limit"=w1676, "dBc Applied?"=w1675) -> (w1681:T3)
                n904 = Build Array (concatenate)(w1684, w1683) -> (w1682:T1)
                n905 = Build Array (concatenate)(w1679, w1681) -> (w1678:T1)
              }
              n906 = Build Array (concatenate)(w1671, T3 {"Freq"=26500.0, "Limit"=-30.0, "dBc Applied?"=FALSE} ("Mask Table")) -> (w1669:T1)
              n907 = Build Array (concatenate)(w1638, T3 {"Freq"=26500.0, "Limit"=-30.0, "dBc Applied?"=FALSE} ("Mask Table")) -> (w1637:T1)
            }
            frame 102 {
              w1693 = T1 [{"Freq"=0.0, "Limit"=-30.0, "dBc Applied?"=FALSE}] ("value")
              n908 = Unbundle By Name(w1720) -> ("BW_N"=w1701:dbl)
              n909 = Multiply(x=1.5, y=w1701) -> (x*y=w1698:dbl)
              n910 = Subtract(x=w1699, y=w1698) -> (x-y=w1725:dbl)
              n911 = Subtract(x=w1699, y=w1701) -> (x-y=w1719:dbl)
              n912 = Subtract(x=w1699, y=280.0) -> (x-y=w1718:dbl)
              n913 = Subtract(x=w1699, y=160.0) -> (x-y=w1714:dbl)
              n914 = Subtract(x=w1699, y=40.0) -> (x-y=w1708:dbl)
              n915 = Subtract(x=w1699, y=80.0) -> (x-y=w1712:dbl)
              n916 = Subtract(x=w1699, y=63.88) -> (x-y=w1709:dbl)
              n917 = Add(x=w1699, y=80.0) -> (x+y=w1705:dbl)
              n918 = Add(x=w1699, y=200.0) -> (x+y=w1702:dbl)
              n919 = Add(x=w1699, y=w1701) -> (x+y=w1700:dbl)
              n920 = Add(x=w1699, y=w1698) -> (x+y=w1697:dbl)
              n921 = Decrement(x=w1714) -> (x-1=w1715:dbl)
              n922 = Increment(x=w1712) -> (x+1=w1711:dbl)
              n923 = Increment(x=w1705) -> (x+1=w1704:dbl)
              n924 = Decrement(x=w1708) -> (x-1=w1707:dbl)
              n925 = Build Array(w1725, w1719, w1718, w1715, w1714, w1712, w1711, w1709, w1707, w1708, w1705, w1704, w1702, w1700, w1697) -> (w1724:dbl[])
              n926 = for {
                tunnel: w1724 -> [w1729] mode=indexing
                tunnel: dbl[] [-30.0, -30.0, -30.0, -20.0, 0.0, 0.0, -20.0, -21.94, -20.0, 0.0, 0.0, -20.0, -30.0, -30.0, -30.0] -> [w1738] mode=indexing
                tunnel: bool[] [FALSE, FALSE, FALSE, TRUE, TRUE, TRUE, TRUE, TRUE, TRUE, TRUE, TRUE, TRUE, FALSE, FALSE, FALSE] -> [w1737] mode=indexing
                shift-right: [w1734] -> w1723
                shift-left: w1693 -> [w1736]
                shift-right: [w1730] -> w1689
                shift-left: w1693 -> [w1731]
                tunnel: dbl[] [-30.0, -30.0, -30.0, -30.0, 0.0, 0.0, -20.0, -21.94, -20.0, 0.0, 0.0, -30.0, -30.0, -30.0, -30.0] -> [w1728] mode=indexing
                tunnel: bool[] [FALSE, FALSE, FALSE, FALSE, TRUE, TRUE, TRUE, TRUE, TRUE, TRUE, TRUE, FALSE, FALSE, FALSE, FALSE] -> [w1727] mode=indexing
                n927 = Bundle By Name(cluster=T3 {"Freq"=0.0, "Limit"=0.0, "dBc Applied?"=FALSE} ("Mask Table"), "Freq"=w1729, "Limit"=w1738, "dBc Applied?"=w1737) -> (w1735:T3)
                n928 = Bundle By Name(cluster=T3 {"Freq"=0.0, "Limit"=0.0, "dBc Applied?"=FALSE} ("Mask Table"), "Freq"=w1729, "Limit"=w1728, "dBc Applied?"=w1727) -> (w1733:T3)
                n929 = Build Array (concatenate)(w1736, w1735) -> (w1734:T1)
                n930 = Build Array (concatenate)(w1731, w1733) -> (w1730:T1)
              }
              n931 = Build Array (concatenate)(w1723, T3 {"Freq"=26500.0, "Limit"=-30.0, "dBc Applied?"=FALSE} ("Mask Table")) -> (w1721:T1)
              n932 = Build Array (concatenate)(w1689, T3 {"Freq"=26500.0, "Limit"=-30.0, "dBc Applied?"=FALSE} ("Mask Table")) -> (w1688:T1)
            }
            frame 103 {
              w1745 = T1 [{"Freq"=0.0, "Limit"=-30.0, "dBc Applied?"=FALSE}] ("value")
              n933 = Unbundle By Name(w1772) -> ("BW_N"=w1753:dbl)
              n934 = Multiply(x=1.5, y=w1753) -> (x*y=w1750:dbl)
              n935 = Subtract(x=w1751, y=w1750) -> (x-y=w1777:dbl)
              n936 = Subtract(x=w1751, y=w1753) -> (x-y=w1771:dbl)
              n937 = Subtract(x=w1751, y=280.0) -> (x-y=w1770:dbl)
              n938 = Subtract(x=w1751, y=160.0) -> (x-y=w1766:dbl)
              n939 = Subtract(x=w1751, y=0.0) -> (x-y=w1760:dbl)
              n940 = Subtract(x=w1751, y=40.0) -> (x-y=w1764:dbl)
              n941 = Subtract(x=w1751, y=16.12) -> (x-y=w1761:dbl)
              n942 = Add(x=w1751, y=80.0) -> (x+y=w1757:dbl)
              n943 = Add(x=w1751, y=200.0) -> (x+y=w1754:dbl)
              n944 = Add(x=w1751, y=w1753) -> (x+y=w1752:dbl)
              n945 = Add(x=w1751, y=w1750) -> (x+y=w1749:dbl)
              n946 = Decrement(x=w1766) -> (x-1=w1767:dbl)
              n947 = Increment(x=w1764) -> (x+1=w1763:dbl)
              n948 = Increment(x=w1757) -> (x+1=w1756:dbl)
              n949 = Decrement(x=w1760) -> (x-1=w1759:dbl)
              n950 = Build Array(w1777, w1771, w1770, w1767, w1766, w1764, w1763, w1761, w1759, w1760, w1757, w1756, w1754, w1752, w1749) -> (w1776:dbl[])
              n951 = for {
                tunnel: w1776 -> [w1781] mode=indexing
                tunnel: dbl[] [-30.0, -30.0, -30.0, -20.0, 0.0, 0.0, -20.0, -21.94, -20.0, 0.0, 0.0, -20.0, -30.0, -30.0, -30.0] -> [w1790] mode=indexing
                tunnel: bool[] [FALSE, FALSE, FALSE, TRUE, TRUE, TRUE, TRUE, TRUE, TRUE, TRUE, TRUE, TRUE, FALSE, FALSE, FALSE] -> [w1789] mode=indexing
                shift-right: [w1786] -> w1775
                shift-left: w1745 -> [w1788]
                shift-right: [w1782] -> w1741
                shift-left: w1745 -> [w1783]
                tunnel: dbl[] [-30.0, -30.0, -30.0, -30.0, 0.0, 0.0, -20.0, -21.94, -20.0, 0.0, 0.0, -30.0, -30.0, -30.0, -30.0] -> [w1780] mode=indexing
                tunnel: bool[] [FALSE, FALSE, FALSE, FALSE, TRUE, TRUE, TRUE, TRUE, TRUE, TRUE, TRUE, FALSE, FALSE, FALSE, FALSE] -> [w1779] mode=indexing
                n952 = Bundle By Name(cluster=T3 {"Freq"=0.0, "Limit"=0.0, "dBc Applied?"=FALSE} ("Mask Table"), "Freq"=w1781, "Limit"=w1790, "dBc Applied?"=w1789) -> (w1787:T3)
                n953 = Bundle By Name(cluster=T3 {"Freq"=0.0, "Limit"=0.0, "dBc Applied?"=FALSE} ("Mask Table"), "Freq"=w1781, "Limit"=w1780, "dBc Applied?"=w1779) -> (w1785:T3)
                n954 = Build Array (concatenate)(w1788, w1787) -> (w1786:T1)
                n955 = Build Array (concatenate)(w1783, w1785) -> (w1782:T1)
              }
              n956 = Build Array (concatenate)(w1775, T3 {"Freq"=26500.0, "Limit"=-30.0, "dBc Applied?"=FALSE} ("Mask Table")) -> (w1773:T1)
              n957 = Build Array (concatenate)(w1741, T3 {"Freq"=26500.0, "Limit"=-30.0, "dBc Applied?"=FALSE} ("Mask Table")) -> (w1740:T1)
            }
            frame 1100 {
              w1797 = T1 [{"Freq"=0.0, "Limit"=-30.0, "dBc Applied?"=FALSE}] ("value")
              n958 = Unbundle By Name(w1824) -> ("BW_N"=w1805:dbl)
              n959 = Multiply(x=1.5, y=w1805) -> (x*y=w1802:dbl)
              n960 = Subtract(x=w1803, y=w1802) -> (x-y=w1829:dbl)
              n961 = Subtract(x=w1803, y=w1805) -> (x-y=w1823:dbl)
              n962 = Subtract(x=w1803, y=280.0) -> (x-y=w1822:dbl)
              n963 = Subtract(x=w1803, y=160.0) -> (x-y=w1818:dbl)
              n964 = Add(x=w1803, y=40.0) -> (x+y=w1812:dbl)
              n965 = Subtract(x=w1803, y=0.0) -> (x-y=w1816:dbl)
              n966 = Subtract(x=w1803, y=-31.63) -> (x-y=w1813:dbl)
              n967 = Add(x=w1803, y=80.0) -> (x+y=w1809:dbl)
              n968 = Add(x=w1803, y=200.0) -> (x+y=w1806:dbl)
              n969 = Add(x=w1803, y=w1805) -> (x+y=w1804:dbl)
              n970 = Add(x=w1803, y=w1802) -> (x+y=w1801:dbl)
              n971 = Decrement(x=w1818) -> (x-1=w1819:dbl)
              n972 = Increment(x=w1816) -> (x+1=w1815:dbl)
              n973 = Increment(x=w1809) -> (x+1=w1808:dbl)
              n974 = Decrement(x=w1812) -> (x-1=w1811:dbl)
              n975 = Build Array(w1829, w1823, w1822, w1819, w1818, w1816, w1815, w1813, w1811, w1812, w1809, w1808, w1806, w1804, w1801) -> (w1828:dbl[])
              n976 = for {
                tunnel: w1828 -> [w1833] mode=indexing
                tunnel: dbl[] [-30.0, -30.0, -30.0, -20.0, 0.0, 0.0, -20.0, -21.94, -20.0, 0.0, 0.0, -20.0, -30.0, -30.0, -30.0] -> [w1842] mode=indexing
                tunnel: bool[] [FALSE, FALSE, FALSE, TRUE, TRUE, TRUE, TRUE, TRUE, TRUE, TRUE, TRUE, TRUE, FALSE, FALSE, FALSE] -> [w1841] mode=indexing
                shift-right: [w1838] -> w1827
                shift-left: w1797 -> [w1840]
                shift-right: [w1834] -> w1793
                shift-left: w1797 -> [w1835]
                tunnel: dbl[] [-30.0, -30.0, -30.0, -30.0, 0.0, 0.0, -20.0, -21.94, -20.0, 0.0, 0.0, -30.0, -30.0, -30.0, -30.0] -> [w1832] mode=indexing
                tunnel: bool[] [FALSE, FALSE, FALSE, FALSE, TRUE, TRUE, TRUE, TRUE, TRUE, TRUE, TRUE, FALSE, FALSE, FALSE, FALSE] -> [w1831] mode=indexing
                n977 = Bundle By Name(cluster=T3 {"Freq"=0.0, "Limit"=0.0, "dBc Applied?"=FALSE} ("Mask Table"), "Freq"=w1833, "Limit"=w1842, "dBc Applied?"=w1841) -> (w1839:T3)
                n978 = Bundle By Name(cluster=T3 {"Freq"=0.0, "Limit"=0.0, "dBc Applied?"=FALSE} ("Mask Table"), "Freq"=w1833, "Limit"=w1832, "dBc Applied?"=w1831) -> (w1837:T3)
                n979 = Build Array (concatenate)(w1840, w1839) -> (w1838:T1)
                n980 = Build Array (concatenate)(w1835, w1837) -> (w1834:T1)
              }
              n981 = Build Array (concatenate)(w1827, T3 {"Freq"=26500.0, "Limit"=-30.0, "dBc Applied?"=FALSE} ("Mask Table")) -> (w1825:T1)
              n982 = Build Array (concatenate)(w1793, T3 {"Freq"=26500.0, "Limit"=-30.0, "dBc Applied?"=FALSE} ("Mask Table")) -> (w1792:T1)
            }
            frame 10103 {
              w1849 = T1 [{"Freq"=0.0, "Limit"=-30.0, "dBc Applied?"=FALSE}] ("value")
              n983 = Unbundle By Name(w1876) -> ("BW_N"=w1857:dbl)
              n984 = Multiply(x=1.5, y=w1857) -> (x*y=w1854:dbl)
              n985 = Subtract(x=w1855, y=w1854) -> (x-y=w1881:dbl)
              n986 = Subtract(x=w1855, y=w1857) -> (x-y=w1875:dbl)
              n987 = Subtract(x=w1855, y=200.0) -> (x-y=w1874:dbl)
              n988 = Subtract(x=w1855, y=80.0) -> (x-y=w1870:dbl)
              n989 = Add(x=w1855, y=0.0) -> (x+y=w1864:dbl)
              n990 = Subtract(x=w1855, y=40.0) -> (x-y=w1868:dbl)
              n991 = Subtract(x=w1855, y=31.63) -> (x-y=w1865:dbl)
              n992 = Add(x=w1855, y=160.0) -> (x+y=w1861:dbl)
              n993 = Add(x=w1855, y=280.0) -> (x+y=w1858:dbl)
              n994 = Add(x=w1855, y=w1857) -> (x+y=w1856:dbl)
              n995 = Add(x=w1855, y=w1854) -> (x+y=w1853:dbl)
              n996 = Decrement(x=w1870) -> (x-1=w1871:dbl)
              n997 = Increment(x=w1868) -> (x+1=w1867:dbl)
              n998 = Increment(x=w1861) -> (x+1=w1860:dbl)
              n999 = Decrement(x=w1864) -> (x-1=w1863:dbl)
              n1000 = Build Array(w1881, w1875, w1874, w1871, w1870, w1868, w1867, w1865, w1863, w1864, w1861, w1860, w1858, w1856, w1853) -> (w1880:dbl[])
              n1001 = for {
                tunnel: w1880 -> [w1885] mode=indexing
                tunnel: dbl[] [-30.0, -30.0, -30.0, -20.0, 0.0, 0.0, -20.0, -21.94, -20.0, 0.0, 0.0, -20.0, -30.0, -30.0, -30.0] -> [w1894] mode=indexing
                tunnel: bool[] [FALSE, FALSE, FALSE, TRUE, TRUE, TRUE, TRUE, TRUE, TRUE, TRUE, TRUE, TRUE, FALSE, FALSE, FALSE] -> [w1893] mode=indexing
                shift-right: [w1890] -> w1879
                shift-left: w1849 -> [w1892]
                shift-right: [w1886] -> w1845
                shift-left: w1849 -> [w1887]
                tunnel: dbl[] [-30.0, -30.0, -30.0, -30.0, 0.0, 0.0, -20.0, -21.94, -20.0, 0.0, 0.0, -30.0, -30.0, -30.0, -30.0] -> [w1884] mode=indexing
                tunnel: bool[] [FALSE, FALSE, FALSE, FALSE, TRUE, TRUE, TRUE, TRUE, TRUE, TRUE, TRUE, FALSE, FALSE, FALSE, FALSE] -> [w1883] mode=indexing
                n1002 = Bundle By Name(cluster=T3 {"Freq"=0.0, "Limit"=0.0, "dBc Applied?"=FALSE} ("Mask Table"), "Freq"=w1885, "Limit"=w1894, "dBc Applied?"=w1893) -> (w1891:T3)
                n1003 = Bundle By Name(cluster=T3 {"Freq"=0.0, "Limit"=0.0, "dBc Applied?"=FALSE} ("Mask Table"), "Freq"=w1885, "Limit"=w1884, "dBc Applied?"=w1883) -> (w1889:T3)
                n1004 = Build Array (concatenate)(w1892, w1891) -> (w1890:T1)
                n1005 = Build Array (concatenate)(w1887, w1889) -> (w1886:T1)
              }
              n1006 = Build Array (concatenate)(w1879, T3 {"Freq"=26500.0, "Limit"=-30.0, "dBc Applied?"=FALSE} ("Mask Table")) -> (w1877:T1)
              n1007 = Build Array (concatenate)(w1845, T3 {"Freq"=26500.0, "Limit"=-30.0, "dBc Applied?"=FALSE} ("Mask Table")) -> (w1844:T1)
            }
            frame 11100 {
              w1901 = T1 [{"Freq"=0.0, "Limit"=-30.0, "dBc Applied?"=FALSE}] ("value")
              n1008 = Unbundle By Name(w1928) -> ("BW_N"=w1909:dbl)
              n1009 = Multiply(x=1.5, y=w1909) -> (x*y=w1906:dbl)
              n1010 = Subtract(x=w1907, y=w1906) -> (x-y=w1933:dbl)
              n1011 = Subtract(x=w1907, y=w1909) -> (x-y=w1927:dbl)
              n1012 = Subtract(x=w1907, y=200.0) -> (x-y=w1926:dbl)
              n1013 = Subtract(x=w1907, y=80.0) -> (x-y=w1922:dbl)
              n1014 = Add(x=w1907, y=40.0) -> (x+y=w1916:dbl)
              n1015 = Subtract(x=w1907, y=0.0) -> (x-y=w1920:dbl)
              n1016 = Subtract(x=w1907, y=-16.12) -> (x-y=w1917:dbl)
              n1017 = Add(x=w1907, y=160.0) -> (x+y=w1913:dbl)
              n1018 = Add(x=w1907, y=280.0) -> (x+y=w1910:dbl)
              n1019 = Add(x=w1907, y=w1909) -> (x+y=w1908:dbl)
              n1020 = Add(x=w1907, y=w1906) -> (x+y=w1905:dbl)
              n1021 = Decrement(x=w1922) -> (x-1=w1923:dbl)
              n1022 = Increment(x=w1920) -> (x+1=w1919:dbl)
              n1023 = Increment(x=w1913) -> (x+1=w1912:dbl)
              n1024 = Decrement(x=w1916) -> (x-1=w1915:dbl)
              n1025 = Build Array(w1933, w1927, w1926, w1923, w1922, w1920, w1919, w1917, w1915, w1916, w1913, w1912, w1910, w1908, w1905) -> (w1932:dbl[])
              n1026 = for {
                tunnel: w1932 -> [w1937] mode=indexing
                tunnel: dbl[] [-30.0, -30.0, -30.0, -20.0, 0.0, 0.0, -20.0, -21.94, -20.0, 0.0, 0.0, -20.0, -30.0, -30.0, -30.0] -> [w1946] mode=indexing
                tunnel: bool[] [FALSE, FALSE, FALSE, TRUE, TRUE, TRUE, TRUE, TRUE, TRUE, TRUE, TRUE, TRUE, FALSE, FALSE, FALSE] -> [w1945] mode=indexing
                shift-right: [w1942] -> w1931
                shift-left: w1901 -> [w1944]
                shift-right: [w1938] -> w1897
                shift-left: w1901 -> [w1939]
                tunnel: dbl[] [-30.0, -30.0, -30.0, -30.0, 0.0, 0.0, -20.0, -21.94, -20.0, 0.0, 0.0, -30.0, -30.0, -30.0, -30.0] -> [w1936] mode=indexing
                tunnel: bool[] [FALSE, FALSE, FALSE, FALSE, TRUE, TRUE, TRUE, TRUE, TRUE, TRUE, TRUE, FALSE, FALSE, FALSE, FALSE] -> [w1935] mode=indexing
                n1027 = Bundle By Name(cluster=T3 {"Freq"=0.0, "Limit"=0.0, "dBc Applied?"=FALSE} ("Mask Table"), "Freq"=w1937, "Limit"=w1946, "dBc Applied?"=w1945) -> (w1943:T3)
                n1028 = Bundle By Name(cluster=T3 {"Freq"=0.0, "Limit"=0.0, "dBc Applied?"=FALSE} ("Mask Table"), "Freq"=w1937, "Limit"=w1936, "dBc Applied?"=w1935) -> (w1941:T3)
                n1029 = Build Array (concatenate)(w1944, w1943) -> (w1942:T1)
                n1030 = Build Array (concatenate)(w1939, w1941) -> (w1938:T1)
              }
              n1031 = Build Array (concatenate)(w1931, T3 {"Freq"=26500.0, "Limit"=-30.0, "dBc Applied?"=FALSE} ("Mask Table")) -> (w1929:T1)
              n1032 = Build Array (concatenate)(w1897, T3 {"Freq"=26500.0, "Limit"=-30.0, "dBc Applied?"=FALSE} ("Mask Table")) -> (w1896:T1)
            }
            frame 11101 {
              w1953 = T1 [{"Freq"=0.0, "Limit"=-30.0, "dBc Applied?"=FALSE}] ("value")
              n1033 = Unbundle By Name(w1980) -> ("BW_N"=w1961:dbl)
              n1034 = Multiply(x=1.5, y=w1961) -> (x*y=w1958:dbl)
              n1035 = Subtract(x=w1959, y=w1958) -> (x-y=w1985:dbl)
              n1036 = Subtract(x=w1959, y=w1961) -> (x-y=w1979:dbl)
              n1037 = Subtract(x=w1959, y=200.0) -> (x-y=w1978:dbl)
              n1038 = Subtract(x=w1959, y=80.0) -> (x-y=w1974:dbl)
              n1039 = Add(x=w1959, y=80.0) -> (x+y=w1968:dbl)
              n1040 = Add(x=w1959, y=40.0) -> (x+y=w1972:dbl)
              n1041 = Subtract(x=w1959, y=-63.88) -> (x-y=w1969:dbl)
              n1042 = Add(x=w1959, y=160.0) -> (x+y=w1965:dbl)
              n1043 = Add(x=w1959, y=280.0) -> (x+y=w1962:dbl)
              n1044 = Add(x=w1959, y=w1961) -> (x+y=w1960:dbl)
              n1045 = Add(x=w1959, y=w1958) -> (x+y=w1957:dbl)
              n1046 = Decrement(x=w1974) -> (x-1=w1975:dbl)
              n1047 = Increment(x=w1972) -> (x+1=w1971:dbl)
              n1048 = Increment(x=w1965) -> (x+1=w1964:dbl)
              n1049 = Decrement(x=w1968) -> (x-1=w1967:dbl)
              n1050 = Build Array(w1985, w1979, w1978, w1975, w1974, w1972, w1971, w1969, w1967, w1968, w1965, w1964, w1962, w1960, w1957) -> (w1984:dbl[])
              n1051 = for {
                tunnel: w1984 -> [w1989] mode=indexing
                tunnel: dbl[] [-30.0, -30.0, -30.0, -20.0, 0.0, 0.0, -20.0, -21.94, -20.0, 0.0, 0.0, -20.0, -30.0, -30.0, -30.0] -> [w1998] mode=indexing
                tunnel: bool[] [FALSE, FALSE, FALSE, TRUE, TRUE, TRUE, TRUE, TRUE, TRUE, TRUE, TRUE, TRUE, FALSE, FALSE, FALSE] -> [w1997] mode=indexing
                shift-right: [w1994] -> w1983
                shift-left: w1953 -> [w1996]
                shift-right: [w1990] -> w1949
                shift-left: w1953 -> [w1991]
                tunnel: dbl[] [-30.0, -30.0, -30.0, -30.0, 0.0, 0.0, -20.0, -21.94, -20.0, 0.0, 0.0, -30.0, -30.0, -30.0, -30.0] -> [w1988] mode=indexing
                tunnel: bool[] [FALSE, FALSE, FALSE, FALSE, TRUE, TRUE, TRUE, TRUE, TRUE, TRUE, TRUE, FALSE, FALSE, FALSE, FALSE] -> [w1987] mode=indexing
                n1052 = Bundle By Name(cluster=T3 {"Freq"=0.0, "Limit"=0.0, "dBc Applied?"=FALSE} ("Mask Table"), "Freq"=w1989, "Limit"=w1998, "dBc Applied?"=w1997) -> (w1995:T3)
                n1053 = Bundle By Name(cluster=T3 {"Freq"=0.0, "Limit"=0.0, "dBc Applied?"=FALSE} ("Mask Table"), "Freq"=w1989, "Limit"=w1988, "dBc Applied?"=w1987) -> (w1993:T3)
                n1054 = Build Array (concatenate)(w1996, w1995) -> (w1994:T1)
                n1055 = Build Array (concatenate)(w1991, w1993) -> (w1990:T1)
              }
              n1056 = Build Array (concatenate)(w1983, T3 {"Freq"=26500.0, "Limit"=-30.0, "dBc Applied?"=FALSE} ("Mask Table")) -> (w1981:T1)
              n1057 = Build Array (concatenate)(w1949, T3 {"Freq"=26500.0, "Limit"=-30.0, "dBc Applied?"=FALSE} ("Mask Table")) -> (w1948:T1)
            }
            frame 11102 {
              w2005 = T1 [{"Freq"=0.0, "Limit"=-30.0, "dBc Applied?"=FALSE}] ("value")
              n1058 = Unbundle By Name(w2032) -> ("BW_N"=w2013:dbl)
              n1059 = Multiply(x=1.5, y=w2013) -> (x*y=w2010:dbl)
              n1060 = Subtract(x=w2011, y=w2010) -> (x-y=w2037:dbl)
              n1061 = Subtract(x=w2011, y=w2013) -> (x-y=w2031:dbl)
              n1062 = Subtract(x=w2011, y=200.0) -> (x-y=w2030:dbl)
              n1063 = Subtract(x=w2011, y=80.0) -> (x-y=w2026:dbl)
              n1064 = Add(x=w2011, y=120.0) -> (x+y=w2020:dbl)
              n1065 = Add(x=w2011, y=80.0) -> (x+y=w2024:dbl)
              n1066 = Subtract(x=w2011, y=-111.63) -> (x-y=w2021:dbl)
              n1067 = Add(x=w2011, y=160.0) -> (x+y=w2017:dbl)
              n1068 = Add(x=w2011, y=280.0) -> (x+y=w2014:dbl)
              n1069 = Add(x=w2011, y=w2013) -> (x+y=w2012:dbl)
              n1070 = Add(x=w2011, y=w2010) -> (x+y=w2009:dbl)
              n1071 = Decrement(x=w2026) -> (x-1=w2027:dbl)
              n1072 = Increment(x=w2024) -> (x+1=w2023:dbl)
              n1073 = Increment(x=w2017) -> (x+1=w2016:dbl)
              n1074 = Decrement(x=w2020) -> (x-1=w2019:dbl)
              n1075 = Build Array(w2037, w2031, w2030, w2027, w2026, w2024, w2023, w2021, w2019, w2020, w2017, w2016, w2014, w2012, w2009) -> (w2036:dbl[])
              n1076 = for {
                tunnel: w2036 -> [w2041] mode=indexing
                tunnel: dbl[] [-30.0, -30.0, -30.0, -20.0, 0.0, 0.0, -20.0, -21.94, -20.0, 0.0, 0.0, -20.0, -30.0, -30.0, -30.0] -> [w2050] mode=indexing
                tunnel: bool[] [FALSE, FALSE, FALSE, TRUE, TRUE, TRUE, TRUE, TRUE, TRUE, TRUE, TRUE, TRUE, FALSE, FALSE, FALSE] -> [w2049] mode=indexing
                shift-right: [w2046] -> w2035
                shift-left: w2005 -> [w2048]
                shift-right: [w2042] -> w2001
                shift-left: w2005 -> [w2043]
                tunnel: dbl[] [-30.0, -30.0, -30.0, -30.0, 0.0, 0.0, -20.0, -21.94, -20.0, 0.0, 0.0, -30.0, -30.0, -30.0, -30.0] -> [w2040] mode=indexing
                tunnel: bool[] [FALSE, FALSE, FALSE, FALSE, TRUE, TRUE, TRUE, TRUE, TRUE, TRUE, TRUE, FALSE, FALSE, FALSE, FALSE] -> [w2039] mode=indexing
                n1077 = Bundle By Name(cluster=T3 {"Freq"=0.0, "Limit"=0.0, "dBc Applied?"=FALSE} ("Mask Table"), "Freq"=w2041, "Limit"=w2050, "dBc Applied?"=w2049) -> (w2047:T3)
                n1078 = Bundle By Name(cluster=T3 {"Freq"=0.0, "Limit"=0.0, "dBc Applied?"=FALSE} ("Mask Table"), "Freq"=w2041, "Limit"=w2040, "dBc Applied?"=w2039) -> (w2045:T3)
                n1079 = Build Array (concatenate)(w2048, w2047) -> (w2046:T1)
                n1080 = Build Array (concatenate)(w2043, w2045) -> (w2042:T1)
              }
              n1081 = Build Array (concatenate)(w2035, T3 {"Freq"=26500.0, "Limit"=-30.0, "dBc Applied?"=FALSE} ("Mask Table")) -> (w2033:T1)
              n1082 = Build Array (concatenate)(w2001, T3 {"Freq"=26500.0, "Limit"=-30.0, "dBc Applied?"=FALSE} ("Mask Table")) -> (w2000:T1)
            }
          }
        }
      }
    }
    frame Error {
    }
  }
  "error out" <- w8
  "SA Measurement out" <- w6
  "SEM Upper Mask Table" <- w2
  "SEM Lower Mask Table" <- w1
